vi "GDSIconEditor_CreateVIIcon.vi"(6 "ViRef(IgnoreIfNotWired)":refnum<vi>, 7 "AutomaticUpdateNoQuestionsAsked(False)":bool, 8 "error in (no error)":errorcluster, 9 "Application:Menu Launch:VI":string, 10 "Application:Menu Launch:App":refnum<vi>, 11 "FileNameConverions":T1) -> (0 "error out":errorcluster)   [LabVIEW 2020]
uses:
  <resource>/Framework/Providers/Open_GDS/ClassProviders/Common/LvIcon_class/GDSLvIcon_ColorControl.ctl
  <resource>/Framework/Providers/Open_GDS/ClassProviders/Common/IconEditor/private/GDSIconEditor_FileNameFilter.ctl
  <resource>/Framework/Providers/Open_GDS/ClassProviders/Common/IconEditor/private/GDSIconEditor_ScopeType.ctl
  <vilib>/picture/picture.llb/imagedata.ctl
  <vilib>/Utility/miscctls.llb/LVPoint32TypeDef.ctl
  <resource>/Framework/Providers/Open_GDS/ClassProviders/Provider_LvNativeClass/ClassWriterNative_class/IconSize.ctl
  <resource>/Framework/Providers/Open_GDS/ClassProviders/Common/LvIcon_class/subvis/GDSLvIcon_TextDataType.ctl
  <resource>/Framework/Providers/Open_GDS/ClassProviders/Common/LvIcon_class/GDSLvIcon_WordCompressionType.ctl
  <resource>/Framework/Providers/Open_GDS/ClassProviders/Common/LvIcon_class/GDSLvIcon_TextAlignment.ctl
  <vilib>/event_ctls.llb/lveventtype.ctl
  <vilib>/Utility/miscctls.llb/LVPositionTypeDef.ctl
  <resource>/Framework/Providers/Open_GDS/ClassProviders/Common/IconEditor/private/GDSIconEditor_IconDialog_Input.vi
  <vilib>/Utility/miscctls.llb/LVPointTypeDef.ctl
  <vilib>/Analysis/baseanly.llb/Mean (DBL).vi
  <resource>/Framework/Providers/Open_GDS/ClassProviders/Provider_LvNativeClass/ClassWriterNative_class/ClassWriterNative.lvclass
  <vilib>/Analysis/NI_AALBase.lvlib
panel:
  in  "QuickIcons":u16(ring) items=["<Select an icon>", "Error Wire overlay", "-", "Configure..."]
  in  "ClearIcon":bool
  out "ProductPicture":picture
  out "_IconPreview":picture caption="Icon Preview"
  out "DragIcon":picture
  in  "_MethodIconName":string caption="Body Text"
  in  "FloodFillMask":bool
  out "_IconName":string
  in  "_IconSearchText":string caption="Icon search text"
  in  "_Manage":bool
  in  "_Folders":u16(ring) caption="Folders" items=["<All icons>", "...EW 2020\\resource\\Framework\\Providers\\Icons", "...source\\Framework\\Providers\\Open_GDS\\Glyphs", "...esource\\Framework\\Providers\\Open_GDS\\Icons", "...el.holmstrom\\Documents\\LabVIEW Data\\Glyphs"]
  out "Icons":picture
  in  "_Icons":bool
  in  "_TextAlignment":u16(ring) caption="Text Alignment" items=["Center", "Left", "Right"]
  in  "_IconSize":u16(ring) caption="Icon Size" items=["Full", "1 c-term high", "2 c-term high", "3 c-term high", "4 c-term high"]
  in  "_HelpCreateClass":bool
  out "_FilePrefixFound":string caption="Prefix found"
  in  "_ApplyHeaderToAll":bool caption="Apply this header to all\nVIs/Ctrls in this folder"
  in  "_BodyTextColor":T2 caption="Body Text"
  in  "_BackgroundColor":T2 caption="Body Background"
  in  "_FontCompression":enum16{"Auto", "On", "Off"}(ring) caption="Font Compression"
  in  "_FontCapitalOnly":bool=TRUE caption="Force Capital Letters"
  out "_After":picture caption="New"
  out "_ViNotSavedMessage":string caption="VI not saved. Please select a path!"
  in  "_Cancel":bool
  in  "Accept":bool
  in  "_EditHeader":bool
  in  "_TemplateVI":bool
  in  "_VIPath":path caption="VI Path"
  out "_Before":picture caption="Current"
  out "_Scope":string caption="Visibility"
  in  "_OCR":bool
  in  "_HideHeader":bool=TRUE caption="Force Capital Letters"
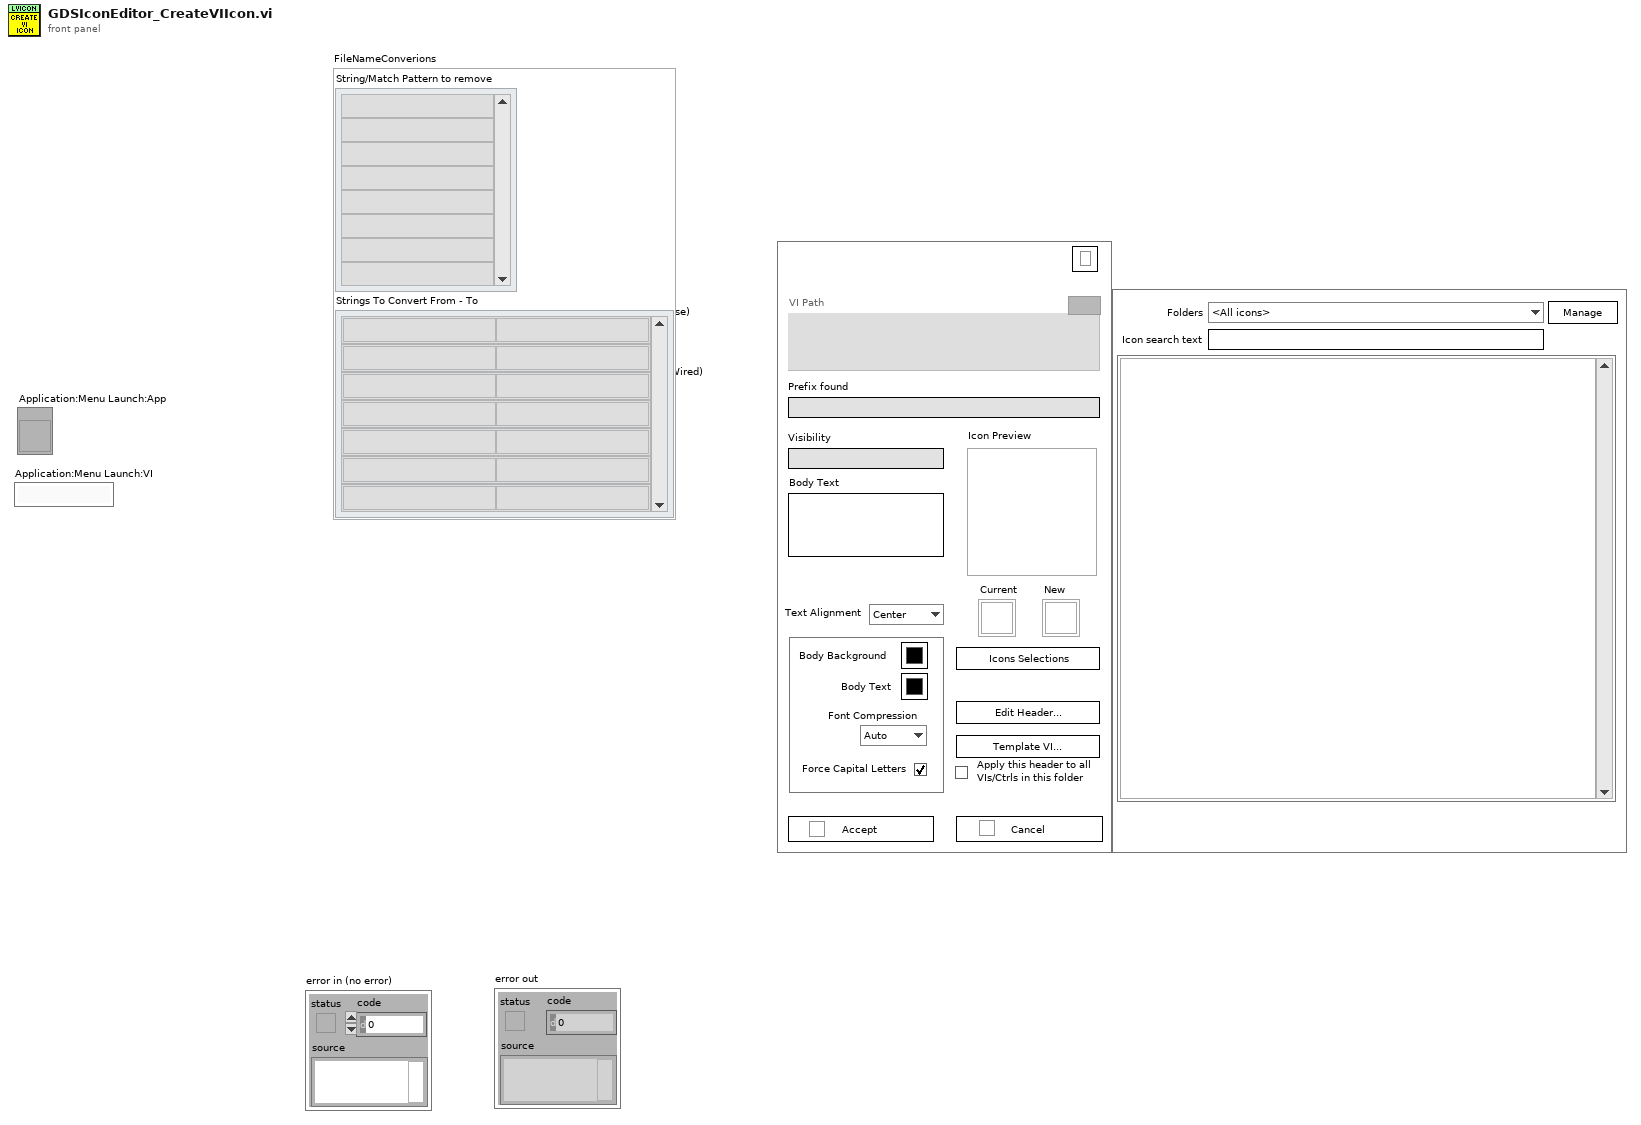
[diagram p1: front panel]
types:
  T1 = typedef "GDSIconEditor_FileNameFilter.ctl" = cluster{"String/Match Pattern to remove":string[], "Strings To Convert From - To":cluster{"From":string, "To":string}[]}
  T2 = typedef "GDSLvIcon_ColorControl.ctl" = cluster{"Decal":bool, "Color":u32}
  T3 = typedef "GDSIconEditor_ScopeType.ctl" = enum16{"Public", "Proteced", "Private"}
  T4 = typedef "imagedata.ctl" = cluster{"image type":i32, "image depth":i32, "image":u8[], "mask":u8[], "colors":u32[], "Rectangle":cluster{"left":i16, "top":i16, "right":i16, "bottom":i16}}
  T5 = typedef "LVPoint32TypeDef.ctl" = cluster{"Horizontal":i32, "Vertical":i32}
  T6 = cluster{"License key":string, "Key info":string, "Prefix":string, "Header exists":bool, "Separator":string, "Folder":path, "VIs":path[], "VI Path":path, "VI exist":bool, "VI name":string, "Icon exist":bool, "ViRef":refnum<vi>, "LibraryRef":refnum<vi>, "Scope":T3, "FrameColor":u32, "Frame thickness":i32, "HeaderIcon":u8[][], "BodyIconHeight":i32, "BodyIconWidth":i32, "IconOut":u8[][], "AppRef":refnum<vi>, "Counter":i32, "Text1":string, "Text2":string, "Text0":string, "Type":enum16{"LvClass", "Library", "X-Control"}, "ConnectorPaneHeight":i32[], "StartRow":i32, "StartIconSize":u16, "Offset":cluster{"X":i32, "Y":i32}, "OldOffset":cluster{"X":i32, "Y":i32}, "Icons":T4[], "IconPos":cluster{"left":i16, "top":i16, "right":i16, "bottom":i16}[], "IconSelected":i32, "BgIcon":u8[][], "BgIconOffset":cluster{"X":i32, "Y":i32}, "Folders":path[], "DraggingIcon":bool, "BodyIcon":u8[][], "BgIconMask":u8[], "HeaderBkColor":u32, "CurrentIcon":cluster{"BgIcon":u8[][], "BgIconOffset":cluster{"X":i32, "Y":i32}, "BgIconMask":u8[], "ColorsOkayforiconToBeOnTopOf":u8[]}, "Moving":bool, "IconDropped":i32, "StartMethodName":string, "DraggingText":bool, "TextBounds":cluster{"FirstRow":i32, "FirstColumn":i32, "LastRow":i32, "LastColumn":i32}, "StartTextDraggingPos":T5, "NoControlsToMove":bool, "LayoutChangeExist":bool, "IconNames":string[], "IconPaths":cluster{i32, "path out":path}[], "Library":bool, "ClassBodyIcon":string, "FirstTime":bool, "TermWindowOpen":bool, "RowStart(0)":i32, "ImageRows(32)":i32, "Splitter0px":bool}
  T7 = typedef "LVBoundsTypeDef.ctl" = cluster{"Width":u32, "Height":u32}
  T8 = typedef "LVRectTypeDef.ctl" = cluster{"Left":i16, "Top":i16, "Right":i16, "Bottom":i16}
  T9 = typedef "ClassWriterNative.lvclass/IconSize.ctl" = enum16{"Full", "1 c-term high", "2 c-term high", "3 c-term high"}
  T10 = typedef "GDSLvIcon_TextDataType.ctl" = cluster{"Text":string, "Allow Only Capital Chars":bool, "Compression":T11, "Alignment":T12}
  T11 = typedef "GDSLvIcon_WordCompressionType.ctl" = enum16{"Auto", "On", "Off"}
  T12 = typedef "GDSLvIcon_TextAlignment.ctl" = enum16{"Center", "Left", "Right"}
  T13 = cluster{"BgIcon":u8[][], "BgIconOffset":cluster{"X":i32, "Y":i32}, "BgIconMask":u8[], "ColorsOkayforiconToBeOnTopOf":u8[]}
  T14 = typedef "lveventtype.ctl" = enum32{"Null", "Timeout", "Annotation Menu Selection", "Annotation Menu Selection?", "App Instance Close", "App Instance Close?", "Autoscale Range Change", "Bookmark Info Change", "Cell Edit", "Cell Edit?", "Cursor Grab", "Cursor Grab?", "Cursor Menu Selection", "Cursor Menu Selection?", "Cursor Move", "Cursor Release", "Data Change", "Direction Change", "Display State Change", "Drag Ended", "Drag Enter", "Drag Leave", "Drag Over", "Drag Source Update", "Drag Starting", "Drag Starting?", "Drop", "Exec State Change", "Key Down", "Key Down?", "Key Repeat", "Key Repeat?", "Key Up", "Listbox Double Click", "Menu Activation?", "Menu Selection (App)", "Menu Selection? (App)", "Menu Selection (User)", "Mouse Down", "Mouse Down?", "Mouse Enter", "Mouse Leave", "Mouse Move", "Mouse Up", "Mouse Wheel", "NI Security User Change (App)", "Pane Size", "Panel Close", "Panel Close?", "Panel Resize", "Plot Attribute Change", "Scale Range Change", "Shortcut Menu Activation?", "Shortcut Menu Selection (App)", "Shortcut Menu Selection? (App)", "Shortcut Menu Selection (User)", "Tree Double Click", "Tree Drag", "Tree Drag?", "Tree Drop", "Tree Drop?", "Tree Item Close", "Tree Item Close?", "Tree Item Open", "Tree Item Open?", "User Event", "Value Change"}
  T15 = typedef "LVPositionTypeDef.ctl" = cluster{"Left":i32, "Top":i32}
  T16 = typedef "GDSIconEditor_IconDialog_Input.vi" = cluster{"HeaderIcon":u8[][], "RowStart(0)":i32, "ImageRows(32)":i32, "FrameThickness(1)":u32, "FrameColor":u32, "IconTextDataType":T10, "BodyTextColor":u32, "BodyBackgroundColor":u32, "BodyIconHeight":i32, "BodyIconWidth":i32, "HeaderBackgroundColor":u32, "BodyIcon":u8[][], "Offset":cluster{"X":i32, "Y":i32}, "CurrentIcon":cluster{"BgIcon":u8[][], "BgIconOffset":cluster{"X":i32, "Y":i32}, "BgIconMask":u8[], "ColorsOkayforiconToBeOnTopOf":u8[]}}
  T17 = typedef "LVPointTypeDef.ctl" = cluster{"Horizontal":i16, "Vertical":i16}
  T18 = enum32{"invalid scope", "public", "private", "protected", "community"}
  T19 = typedef "Librarian File Info Out.ctl" = cluster{"creation date":u32, "last mod date":u32, "type":string, "creator":string, "LV version":i32, "size":i32, "top level":bool}
  T20 = enum32{"invalid VI type", "Standard VI", "Control VI", "Global VI", "Polymorphic VI", "Configuration VI", "SubSystem", "Facade VI", "Method VI", "Statechart Diagram VI"}
  T21 = typedef "GDSLvClass_IconSettingsType.ctl" = cluster{"Frame":u32, "Frame thickness":u8, "Header Background":u32, "Header Text":u32, "ColorPublic":u32, "ColorProtected":u32, "ColorPrivate":u32, "Body Text":u32, "ClassBodyIcon":string}
  T22 = cluster{"CtrlRef":refnum<vi>, "BeforeTerminalIndex":i32, "AfterTerminalIndex":i32}[]
  T23 = cluster{"FirstRow":i32, "FirstColumn":i32, "LastRow":i32, "LastColumn":i32}
  T24 = typedef "ColorControl.ctl" = cluster{"Decal":bool, "Color":u32}
  T25 = typedef "LVMouseTypeDef.ctl" = cluster{"Mouse Position":cluster{"X":i32, "Y":i32}, "Mouse Modifiers":cluster{"Button Down":bool, "Shift Mod":bool, "Menu Mod":bool, "Option Mod":bool}}
  T26 = cluster{"left":i16, "top":i16, "right":i16, "bottom":i16}[]
  T27 = typedef "eventvkey.ctl" = enum16{"ASCII", "Enter", "Return", "Shift", "Ctrl", "Alt", "Cmd", "Opt", "Caps", "NumLock", "Clear", "Break", "Up", "Down", "Left", "Right", "Insert", "Delete", "Home", "End", "PageUp", "PageDown", "Escape", "Help", "Pause", "ScrollLock", "F1", "F2", "F3", "F4", "F5", "F6", "F7", "F8", "F9", "F10", "F11", "F12", "F13", "F14", "F15", "F16", "F17", "F18", "F19", "F20", "F21", "F22", "F23", "F24", "Play", "VolumeUp", "VolumeDown", "Mute", "Two Byte Char"}
  T28 = cluster{"Shift":bool, "Ctrl":bool, "Alt":bool, "Cmd":bool, "Opt":bool}
  T29 = cluster{"left":i16, "top":i16, "right":i16, "bottom":i16}
  T30 = enum32{"existing file", "new file", "new or existing file", "existing dir", "new dir", "new or existing dir", "existing file (use LLBs)", "new file (use LLBs)", "new or existing file (use LLBs)", "new or existing file or directory (use LLBs)", "existing dir (use LLBs)", "new dir (use LLBs)", "new or existing dir (use LLBs)", "existing file or dir", "new file or dir", "new or existing file or dir", "existing file or dir (use LLBs)", "new file or dir (use LLBs)"}
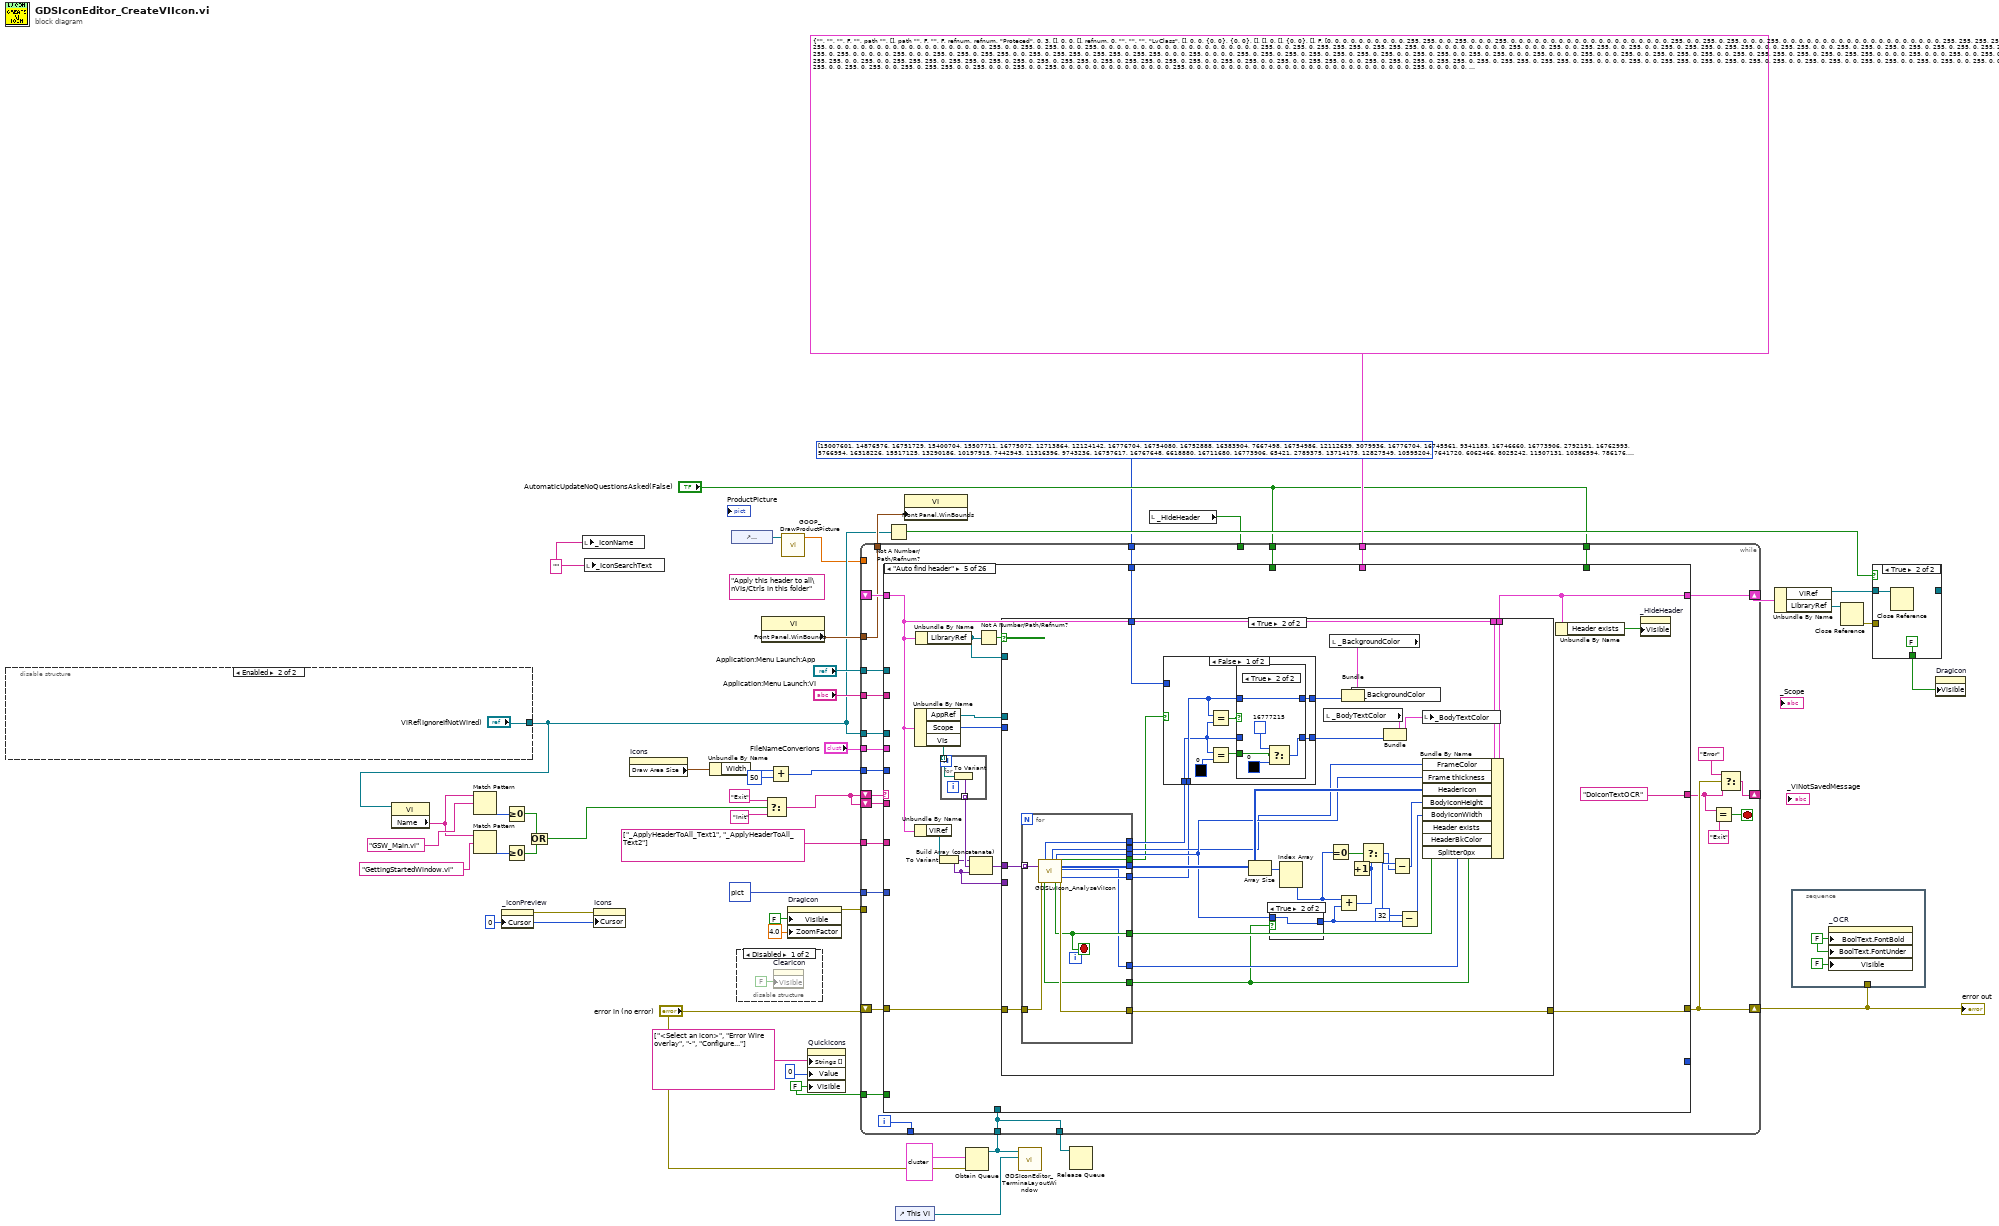
[diagram p0: block diagram]
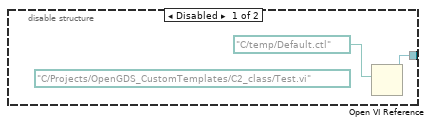
[diagram p3: hidden frame]
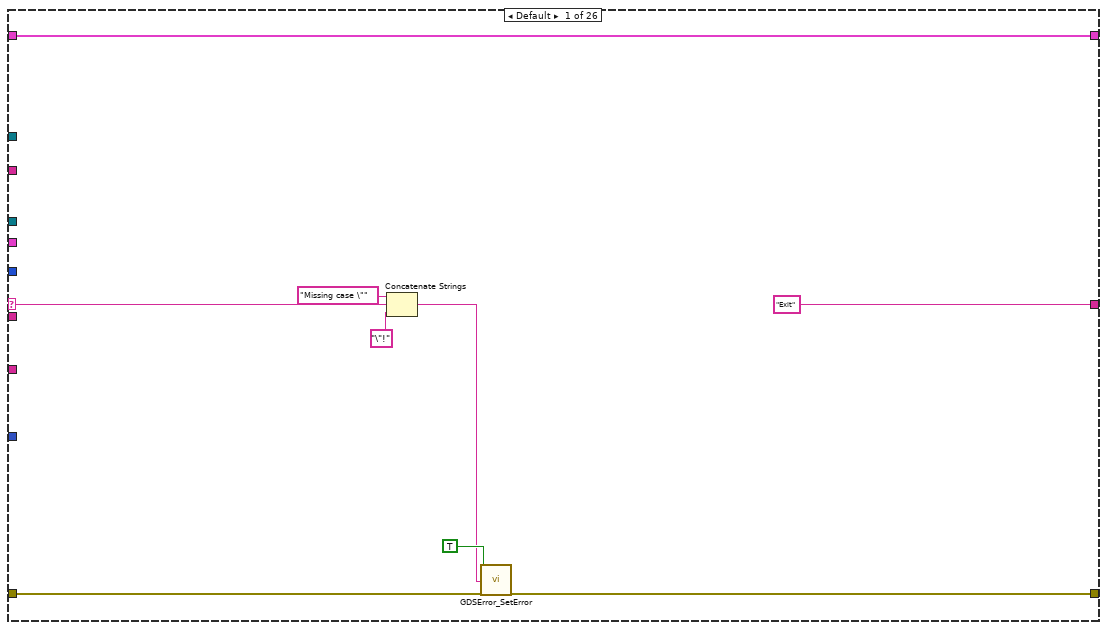
[diagram p5: hidden frame]
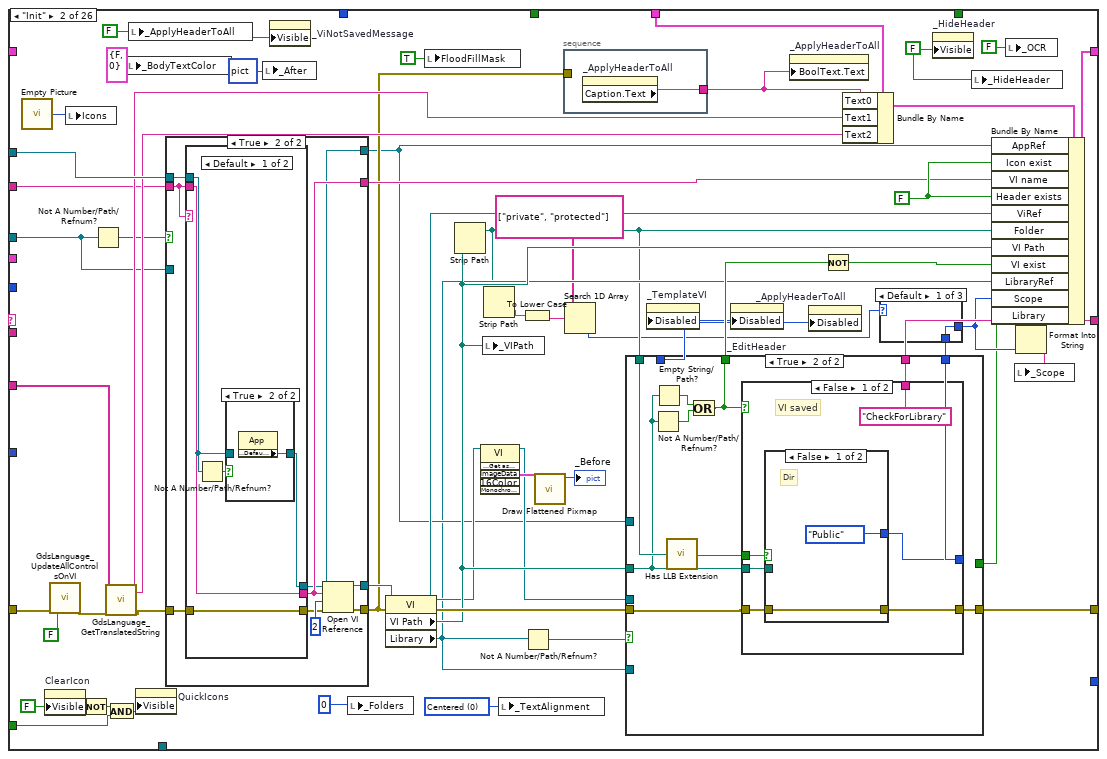
[diagram p6: hidden frame]
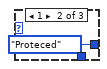
[diagram p7: hidden frame]
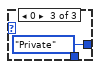
[diagram p8: hidden frame]
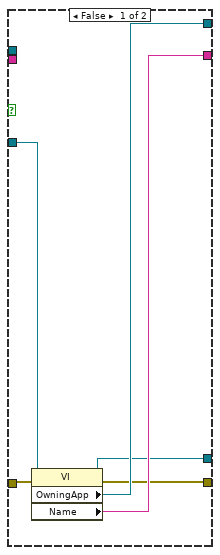
[diagram p9: hidden frame]
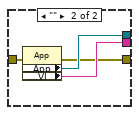
[diagram p11: hidden frame]
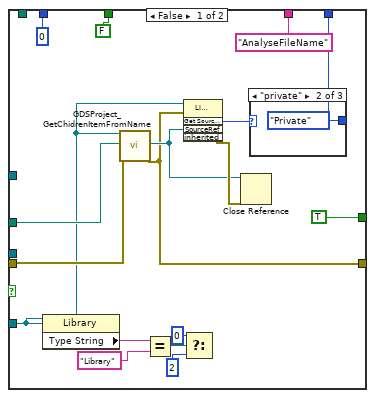
[diagram p12: hidden frame]
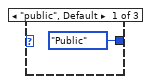
[diagram p13: hidden frame]
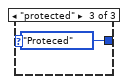
[diagram p14: hidden frame]
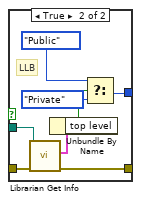
[diagram p15: hidden frame]
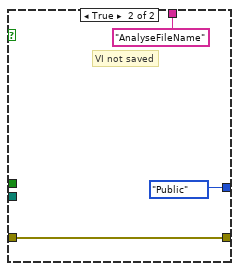
[diagram p16: hidden frame]
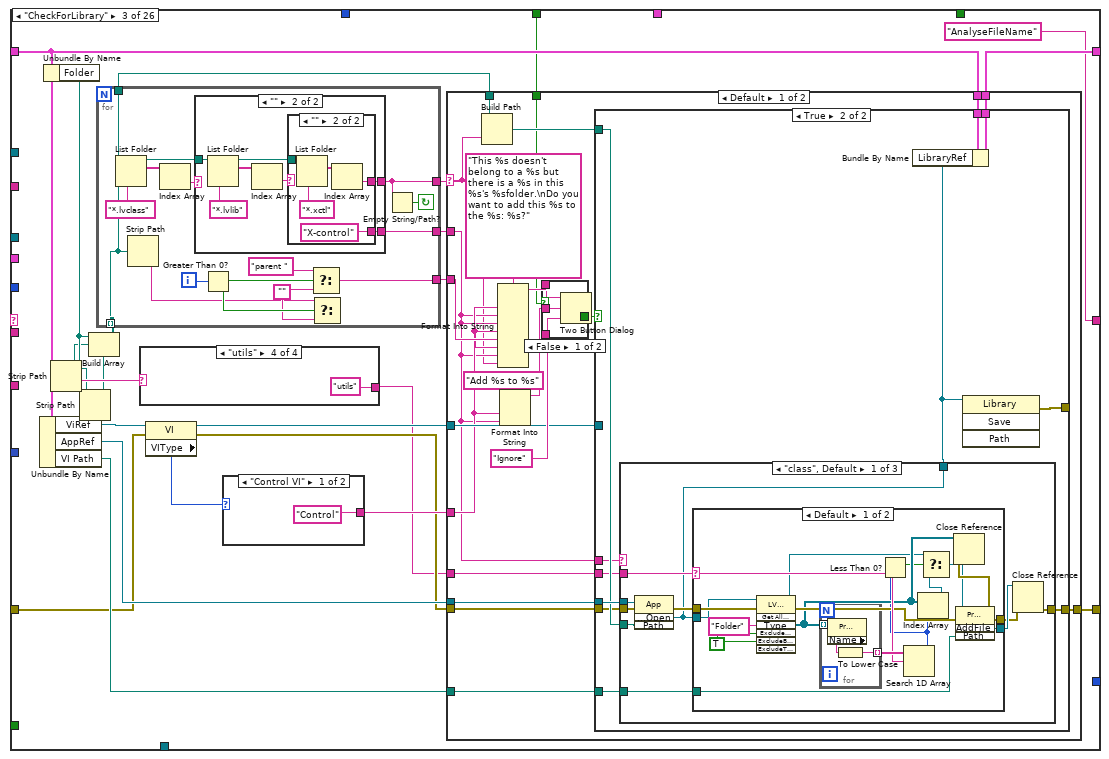
[diagram p17: hidden frame]
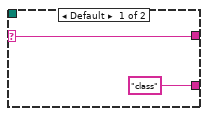
[diagram p18: hidden frame]
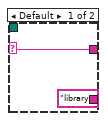
[diagram p19: hidden frame]
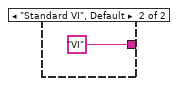
[diagram p20: hidden frame]
diagram:
  w1 = FALSE ("Visible")
  w24 = "" ("_IconSearchText")
  w27 = 0 ("Cursor")
  (unwired) "Apply this header to all\nVIs/Ctrls in this folder" ("Caption.Text")
  n1 = disable-structure shown="Enabled" {
    disable-tunnel: [w52 "ViRef(IgnoreIfNotWired)"] -> w22
    frame Disabled {
      (unwired) path "C:/Projects/OpenGDS_CustomTemplates/C2_class/Test.vi" ("Folder Path")
      n2 = Open VI Reference(vi path=path "C:/temp/Default.ctl" ("Folder Path")) -> (vi reference=w52:refnum<vi>)  [unwired: 5 in, 1 out]
    }
    frame Enabled {
    }
  }
  n3 = property class="VI"(reference=w22) -> ("Name"=w11:string)  [unwired: 1 in, 2 out]
  n4 = Match Pattern(string=w11, regular expression="GSW_Main.vi" ("y")) -> (offset past match=w13:i32)  [unwired: 1 in, 3 out]
  n5 = Match Pattern(string=w11, regular expression="GettingStartedWindow.vi" ("y")) -> (offset past match=w12:i32)  [unwired: 1 in, 3 out]
  n6 = property on="_IconPreview" class="Pict"("Cursor"=w27) -> (error out=w26:errorcluster)  [unwired: 2 in, 1 out]
  n7 = Greater Or Equal To 0?(x=w13) -> (x >= 0?=w8:bool)
  n8 = Greater Or Equal To 0?(x=w12) -> (x >= 0?=w9:bool)
  n9 = Or(x=w8, y=w9) -> (x .or. y?=w18:bool)
  n10 = local write "_IconName"(w24) -> ()
  n11 = local write "_IconSearchText"(w24) -> ()
  n12 = property on="Icons" class="Pict"(error in=w26, "Cursor"=w27) -> ()  [unwired: 1 in, 2 out]
  n13 = property on="Icons" class="Pict"() -> ("Draw Area Size"=w33:T7)  [unwired: 2 in, 2 out]
  n14 = Unbundle By Name(w33) -> ("Width"=w35:u32)
  n15 = control-ref of="ProductPicture"() -> (w6:refnum<vi>)
  n16 = disable-structure shown="Disabled" {
    frame Disabled {
      n17 = property on="ClearIcon" class="Bool"("Visible"=FALSE) -> ()  [unwired: 2 in, 2 out]
    }
    frame Enabled {
    }
  }
  n18 = property class="VI"() -> ("Front Panel.WinBounds"=w25:T8)  [unwired: 2 in, 2 out]
  n19 = Select(t="Exit", s=w18, f="Init") -> (s? t:f=w19:string)
  n20 = Add(x=w35, y=u32 50) -> (x+y=w34:u32)
  n21 = call <resource>:"GOOP_DrawProductPicture.vi"("ProductPictureControl"=w6) -> ("Zoom Factor"=w5:sgl)  [unwired: 10 in]
  n22 = property on="DragIcon" class="Pict"("Visible"=FALSE, "ZoomFactor"=sgl 4.0 ("Zoom Factor")) -> (error out=w30:errorcluster)  [unwired: 2 in, 1 out]
  n23 = property on="QuickIcons" class="Ring (strict)"("Strings []"=string[] ["<Select an icon>", "Error Wire overlay", "-", "Configure..."], "Value"=0, "Visible"=w1) -> ()  [unwired: 2 in, 2 out]
  n24 = Not A Number/Path/Refnum?(number/path/refnum=w22) -> (NaN/Path/Refnum?=w43:bool)
  n25 = control-ref of="This VI"() -> (w37:refnum<vi>)
  n26 = Obtain Queue(element data type=cluster{"Message":string, "Picture":picture} {"Message"="", "Picture"=bytes[0]} ("Message"), error in (no error)="error in (no error)") -> (queue out=w38:refnum<queue>)  [unwired: 3 in, 2 out]
  n27 = call <resource>:"GDSIconEditor_TerminaLayoutWindow.vi"("ViRef"=w37, "ControlQueue"=w38) -> ()  [unwired: 10 in]
  n28 = local read "_HideHeader"() -> (w7:bool)
  n29 = while {
    tunnel: picture bytes[1054] ("Icon not available") -> [w76]
    shift-left: "error in (no error)" -> [w79]
    shift-right: [w71] -> w23
    shift-left: _ -> [w77]
    shift-right: [w78] -> w49
    shift-left: w19 -> [w80]
    shift-right: [w70] -> _
    tunnel: "Application:Menu Launch:App" -> [w75]
    tunnel: "Application:Menu Launch:VI" -> [w74]
    tunnel: T6 {"License key"="", "Key info"="", "Prefix"="", "Header exists"=FALSE, "Separator"="", "Folder"=path "", "VIs"=[], "VI Path"=path "", "VI exist"=FALSE, "VI name"="", "Icon exist"=FALSE, "ViRef"=refnum, "LibraryRef"=refnum, "Scope"=enum."Proteced", "FrameColor"=0, "Frame thickness"=3, "HeaderIcon"=[], "BodyIconHeight"=0, "BodyIconWidth"=0, "IconOut"=[], "AppRef"=refnum, "Counter"=0, "Text1"="", "Text2"="", "Text0"="", "Type"=enum."LvClass", "ConnectorPaneHeight"=[], "StartRow"=0, "StartIconSize"=0, "Offset"={"X"=0, "Y"=0}, "OldOffset"={"X"=0, "Y"=0}, "Icons"=[], "IconPos"=[], "IconSelected"=0, "BgIcon"=[], "BgIconOffset"={"X"=0, "Y"=0}, "Folders"=[], "DraggingIcon"=FALSE, "BodyIcon"=[[0, 0, 0, 0, 0, 0, 0, 0, 0, 0, 255, 255, 0, 0, 255, 0, 0, 0, 255, 0, 0, 0, 0, 0, 0, 0, 0, 0, 0, 0], [0, 0, 0, 0, 0, 0, 0, 0, 0, 255, 0, 0, 255, 0, 255, 0, 0, 0, 255, 0, 0, 0, 0, 0, 0, 0, 0, 0, 0, 0], [0, 0, 0, 0, 0, 0, 0, 0, 0, 255, 255, 255, 255, 0, 255, 0, 0, 0, 255, 0, 0, 0, 0, 0, 0, 0, 0, 0, 0, 0], [0, 0, 0, 0, 0, 0, 0, 0, 0, 255, 0, 0, 255, 0, 255, 0, 0, 0, 255, 0, 0, 0, 0, 0, 0, 0, 0, 0, 0, 0], [0, 0, 0, 0, 0, 0, 0, 0, 0, 255, 0, 0, 255, 0, 255, 255, 255, 0, 255, 255, 255, 0, 0, 0, 0, 0, 0, 0, 0, 0], [0, 0, 255, 0, 0, 0, 255, 0, 0, 255, 255, 0, 0, 255, 0, 0, 255, 0, 255, 255, 0, 255, 255, 0, 0, 0, 255, 255, 0, 0], [0, 255, 0, 255, 0, 255, 0, 255, 0, 255, 0, 255, 0, 255, 255, 0, 255, 0, 255, 0, 0, 255, 0, 255, 0, 255, 0, 0, 0, 0], [0, 255, 0, 0, 0, 255, 0, 255, 0, 255, 255, 0, 0, 255, 0, 255, 255, 0, 255, 255, 0, 255, 255, 0, 0, 0, 255, 0, 0, 0], [0, 255, 0, 255, 0, 255, 0, 255, 0, 255, 0, 255, 0, 255, 0, 0, 255, 0, 255, 0, 0, 255, 0, 255, 0, 0, 0, 255, 0, 0], [0, 0, 255, 0, 0, 0, 255, 0, 0, 255, 0, 255, 0, 255, 0, 0, 255, 0, 255, 255, 0, 255, 0, 255, 0, 255, 255, 0, 0, 0], [0, 255, 0, 0, 0, 255, 0, 0, 255, 0, 0, 255, 0, 255, 0, 0, 255, 0, 255, 255, 0, 0, 255, 0, 0, 255, 255, 255, 0, 255], [255, 0, 255, 0, 255, 0, 255, 0, 255, 255, 0, 255, 0, 255, 255, 0, 255, 0, 255, 0, 0, 255, 0, 255, 0, 0, 255, 0, 0, 255], [255, 0, 0, 0, 255, 0, 255, 0, 255, 0, 255, 255, 0, 255, 0, 255, 255, 0, 255, 255, 0, 255, 0, 0, 0, 0, 255, 0, 0, 255], [255, 0, 255, 0, 255, 0, 255, 0, 255, 0, 0, 255, 0, 255, 0, 0, 255, 0, 255, 0, 0, 255, 0, 255, 0, 0, 255, 0, 0, 255], [0, 255, 0, 0, 0, 255, 0, 0, 255, 0, 0, 255, 0, 255, 0, 0, 255, 0, 255, 255, 0, 0, 255, 0, 0, 0, 255, 0, 0, 255], [0, 0, 0, 0, 0, 0, 0, 0, 0, 0, 0, 0, 0, 0, 255, 0, 0, 0, 0, 0, 0, 0, 0, 0, 0, 0, 0, 0, 0, 0], [0, 0, 0, 0, 0, 0, 0, 0, 0, 0, 0, 0, 0, 255, 0, 0, 0, 0, 0, 0, 0, 0, 0, 0, 0, 0, 0, 0, 0, 0], [0, 0, 0, 0, 0, 0, 0, 0, 0, 0, 0, 0, 0, 255, 255, 0, 0, 0, 0, 0, 0, 0, 0, 0, 0, 0, 0, 0, 0, 0], [0, 0, 0, 0, 0, 0, 0, 0, 0, 0, 0, 0, 0, 255, 0, 255, 0, 0, 0, 0, 0, 0, 0, 0, 0, 0, 0, 0, 0, 0], [0, 0, 0, 0, 0, 0, 0, 0, 0, 0, 0, 0, 0, 0, 255, 0, 0, 0, 0, 0, 0, 0, 0, 0, 0, 0, 0, 0, 0, 0], [0, 0, 0, 0, 0, 0, 0, 0, 0, 0, 0, 0, 0, 0, 0, 0, 0, 0, 0, 0, 0, 0, 0, 0, 0, 0, 0, 0, 0, 0], [0, 0, 0, 0, 0, 0, 0, 0, 0, 0, 0, 0, 0, 0, 0, 0, 0, 0, 0, 0, 0, 0, 0, 0, 0, 0, 0, 0, 0, 0]], "BgIconMask"=[], "HeaderBkColor"=0, "CurrentIcon"={"BgIcon"=[], "BgIconOffset"={"X"=0, "Y"=0}, "BgIconMask"=[], "ColorsOkayforiconToBeOnTopOf"=[]}, "Moving"=FALSE, "IconDropped"=-1, "StartMethodName"="", "DraggingText"=FALSE, "TextBounds"={"FirstRow"=2, "FirstColumn"=1, "LastRow"=6, "LastColumn"=27}, "StartTextDraggingPos"={"Horizontal"=0, "Vertical"=0}, "NoControlsToMove"=FALSE, "LayoutChangeExist"=FALSE, "IconNames"=[], "IconPaths"=[], "Library"=FALSE, "ClassBodyIcon"="", "FirstTime"=TRUE, "TermWindowOpen"=FALSE, "RowStart(0)"=0, "ImageRows(32)"=32, "Splitter0px"=FALSE} ("Local data") -> [w67]
    shift-left: w19 -> [w66]
    tunnel: string[] ["_ApplyHeaderToAll_Text1", "_ApplyHeaderToAll_Text2"] -> [w65]
    tunnel: w22 -> [w64]
    tunnel: w38 -> [w63]
    tunnel: [w63] -> w39
    tunnel: w34 -> [w62]
    tunnel: w25 -> [w61]
    tunnel: [w61] -> w32
    tunnel: w30 -> [_]
    tunnel: [w60] -> _
    tunnel: "AutomaticUpdateNoQuestionsAsked(False)" -> [w59]
    tunnel: "AutomaticUpdateNoQuestionsAsked(False)" -> [w58]
    tunnel: u32[] [15007601, 14876576, 16751729, 15400704, 15507711, 16775072, 12713864, 12124142, 16776704, 16754080, 16752888, 16383904, 7667498, 16754986, 12112639, 3079936, 16776704, 16745561, 9341183, 16746660, 16773906, 2792191, 16762993, 5766954, 16318226, 15517125, 13290186, 10197915, 7442943, 11316396, 9743236, 16757617, 16767648, 6618880, 16711680, 16773906, 65421, 2789375, 13714175, 12827549, 10595204, 7641720, 6062466, 8025242, 11507131, 10386594, 786176, 8584960, 16318208, 16731648, 16755616, 16734715, 14399157, 16754801, 16714752, 10026888, 3524608] -> [w57]
    tunnel: w7 -> [_]
    tunnel: w5 -> [_]
    tunnel: "FileNameConverions" -> [w56]
    tunnel: w1 -> [w55]
    i -> [w60]
    stop <- w73 stop-if-true
    n30 = case shown="\"Auto find header\"" w80 {
      selector: w80 -> [w82 _ _ _ _ _ w824 _ _ w957 _ _ _ w1613 _ _ _ w1794 _ _ _ _ _ _ _ _]
      tunnel: ["Exit" w111 "AnalyseFileName" "Auto find header" "DoIconTextOCR" "DoIconTextOCR_Before" ("t") w819 "Generate icon" "ShowLayoutChange" ("item tag") w976 w1021 w1096 "UpdateIcon" ("y") w1620 "ReadIcons" "Generate icon" "DrawIcons" ("y") "Idle" ("y") "Idle" ("y") "Exit" w1950 "Auto find header" w2015 "Exit" ("y") w2079 "Exit" ("y")] -> w69
      tunnel: w79 -> [w89 w126 w233 w424 w539 w767 w828 w843 w877 w956 w1039 w1067 w1594 w1648 w1680 w1745 w1756 w1804 w1929 w1940 w1961 w2000 w2023 w2048 w2081 w2131]
      tunnel: [w88 w140 w232 w431 w540 w792 w829 w842 w876 w953 w1038 w1066 w1594 w1648 w1679 w1745 w1751 w1806 w1929 w1937 w1962 w2001 w2008 w2047 w2080 w2131] -> w71
      tunnel: [w85 w144 w246 w430 w529 w793 w816 w840 w873 w960 w1024 w1082 w1596 w1617 w1689 w1746 w1761 w1819 w1925 w1941 w1964 w1997 w2011 w2052 w2076 w2130] -> w78
      tunnel: w77 -> [w85 _ w242 w423 w536 w791 w817 w841 w874 w961 w1025 w1083 w1597 w1617 w1690 w1747 w1759 w1807 w1932 w1941 w1963 w2002 w2011 w2052 w2077 w2130]
      tunnel: w76 -> [_ _ _ _ _ _ _ _ _ _ _ _ _ _ _ _ _ _ _ _ _ _ _ _ _ _]
      tunnel: w75 -> [_ w136 _ _ _ _ _ _ _ _ _ _ _ _ _ _ _ _ _ _ _ _ _ _ _ _]
      tunnel: w74 -> [_ w117 _ _ _ _ _ _ _ _ _ _ _ _ _ _ _ _ _ _ _ _ _ _ _ _]
      tunnel: w67 -> [_ w119 _ _ _ _ _ _ _ _ _ _ _ _ _ _ _ _ _ _ _ _ _ _ _ _]
      tunnel: w66 -> [_ _ _ _ _ _ _ _ _ _ _ _ _ _ _ _ _ _ _ _ _ _ _ _ _ w2132]
      tunnel: w65 -> [_ w123 _ _ _ _ _ _ _ _ _ _ _ _ _ _ _ _ _ _ _ _ _ _ _ _]
      tunnel: w64 -> [_ w112 _ _ _ _ _ _ _ _ _ _ _ _ _ _ _ _ _ _ _ _ _ _ _ _]
      tunnel: w63 -> [_ _ _ _ _ _ _ _ _ _ w1037 w1071 _ _ _ _ _ _ _ _ _ _ _ _ _ _]
      tunnel: w62 -> [_ _ _ _ _ _ _ _ _ _ _ w1072 _ _ _ _ _ _ _ _ _ _ _ _ _ _]
      tunnel: [_ _ _ _ _ _ _ _ _ w950 _ _ _ _ _ _ _ _ _ _ _ _ _ _ _ _] -> _
      tunnel: w59 -> [_ _ w224 _ _ _ _ _ _ _ _ _ _ _ _ _ _ _ _ _ _ _ _ _ _ _]
      tunnel: w58 -> [_ _ _ _ _ _ _ _ _ w949 w1020 _ _ _ _ _ _ _ _ _ _ _ _ _ _ _]
      tunnel: w57 -> [_ _ _ _ w527 w760 _ _ _ _ _ _ _ _ _ _ _ _ _ _ _ _ _ _ _ _]
      tunnel: w56 -> [_ _ _ w418 _ _ _ _ _ _ _ _ _ _ _ _ _ _ _ _ _ _ _ _ _ _]
      tunnel: w55 -> [_ w90 _ _ _ _ _ _ _ _ _ w1065 _ _ _ _ _ _ _ _ _ _ _ _ _ _]
      frame Default {
        n31 = Concatenate Strings("Missing case \"" ("source"), w82, "\"!") -> (w81:string)
        n32 = call <resource>:"GDSError_SetError.vi"("status"=TRUE, "source"=w81, "error in (no error)"=w89) -> ("error out"=w88:errorcluster)  [unwired: 16 in]
      }
      frame "Init" {
        w93 = FALSE ("Visible")
        w94 = FALSE ("_OCR")
        w108 = u16 0 items=["Centered", "Left", "Right"] ("_TextAlignment")
        w106 = FALSE ("ApplyToAll")
        w139 = FALSE ("Header exists")
        n33 = call "Empty Picture"() -> ("empty picture"=w105:picture)
        n34 = property on="ClearIcon" class="Bool"("Visible"=w93) -> ()  [unwired: 2 in, 2 out]
        n35 = call <resource>:"GdsLanguage_UpdateAllControlsOnVI.vi"("error in (no error)"=w126, "CreateLanguageFile(Use this to create a languageFile)"=FALSE) -> ("error out"=w124:errorcluster)  [unwired: 16 in, 1 out]
        n36 = local write "Icons"(w105) -> ()
        n37 = Not(x=w93) -> (.not. x?=w92:bool)
        n38 = Not A Number/Path/Refnum?(number/path/refnum=w112) -> (NaN/Path/Refnum?=w114:bool)
        n39 = call <resource>:"GdsLanguage_GetTranslatedString.vi"("StringID(s)"=w123, "error in (no error)"=w124) -> ("FirstStringOut"=w121:string, "SecondStringOut"=w120:string, "error out"=w118:errorcluster)  [unwired: 14 in, 1 out]
        n40 = And(x=w92, y=w90) -> (x .and. y?=w91:bool)
        n41 = local write "_BodyTextColor"(T2 {"Decal"=FALSE, "Color"=0} ("BodyText")) -> ()
        n42 = local write "_ApplyHeaderToAll"(w106) -> ()
        n43 = property on="QuickIcons" class="Ring (strict)"("Visible"=w91) -> ()  [unwired: 2 in, 2 out]
        n44 = case shown="True" w114 {
          tunnel: [w149 w161] -> w143
          tunnel: [w150 w160] -> w138
          tunnel: w136 -> [_ w158]
          tunnel: [w151 w157] -> w113
          tunnel: w118 -> [w153 w156]
          tunnel: w117 -> [_ w155]
          tunnel: [w148 w154] -> w116
          tunnel: w112 -> [w152 _]
          frame False {
            n45 = property class="VI"(reference=w152, error in=w153) -> (reference out=w149:refnum<vi>, error out=w148:errorcluster, "OwningApp"=w151:refnum<vi>, "Name"=w150:string)
          }
          frame True {
            n46 = case shown="Default" w155 {
              tunnel: [w163 w173] -> w157
              tunnel: [w167 w172] -> w160
              tunnel: [w166 w171] -> w159
              tunnel: w156 -> [w166 w170]
              tunnel: w158 -> [w164 _]
              tunnel: w155 -> [w167 _]
              frame Default {
                n47 = Not A Number/Path/Refnum?(number/path/refnum=w164) -> (NaN/Path/Refnum?=w165:bool)
                n48 = case shown="True" w165 {
                  tunnel: w164 -> [w168 _]
                  tunnel: [w168 w169] -> w163
                  frame False {
                  }
                  frame True {
                    n49 = property class="App"() -> ("App.DefaultApplication"=w169:refnum<vi>)  [unwired: 2 in, 2 out]
                  }
                }
              }
              frame "" {
                n50 = property class="App"(error in=w170) -> (error out=w171:errorcluster, "Application:Menu Launch:App"=w173:refnum<vi>, "Application:Menu Launch:VI"=w172:string)  [unwired: 1 in, 1 out]
              }
            }
            n51 = Open VI Reference(application reference (local)=w157, vi path=w160, options=2, error in (no error)=w159) -> (vi reference=w161:refnum<vi>, error out=w154:errorcluster)  [unwired: 2 in]
          }
        }
        n52 = local write "_After"(picture bytes[1054] ("After")) -> ()
        n53 = property on="_ViNotSavedMessage" class="Str"("Visible"=w106) -> ()  [unwired: 2 in, 2 out]
        n54 = local write "_Folders"(0) -> ()
        n55 = property class="VI"(reference=w143, error in=w116) -> (reference out=w130:refnum<vi>, error out=w137:errorcluster, "VI Path"=w135:path, "Library"=w110:refnum<vi>)
        n56 = local write "FloodFillMask"(TRUE ("FloodFillMask")) -> ()
        n57 = Strip Path(path=w135) -> (stripped path=w102:path)  [unwired: 1 out]
        n58 = invoke class="VI" method="VI Icon.Get as Image Data"(reference=w130) -> (reference out=w129:refnum<vi>, "ImageData"=w132:T4)  [unwired: 5 in, 4 out]
        n59 = local write "_VIPath"(w135) -> ()
        n60 = Strip Path(path=w102) -> (name=w101:string)  [unwired: 1 out]
        n61 = local write "_TextAlignment"(w108) -> ()
        n62 = To Lower Case(string=w101) -> (all lower case string=w104:string)
        n63 = Not A Number/Path/Refnum?(number/path/refnum=w110) -> (NaN/Path/Refnum?=w109:bool)
        n64 = call <vilib>:"Draw Flattened Pixmap.vi"("image data"=w132) -> ("new picture"=→"_Before":picture)  [unwired: 8 in]
        n65 = stacked-sequence {
          tunnel: [w174] -> w115
          tunnel: w116 -> [_]
          frame #0 {
            n66 = property on="_ApplyHeaderToAll" class="Bool (strict)"() -> ("Caption.Text"=w174:string)  [unwired: 2 in, 2 out]
          }
        }
        n67 = Search 1D Array(1D array=string[] ["private", "protected"], element=w104) -> (index of element=w100:i32)  [unwired: 1 in]
        n68 = case shown="True" w109 {
          tunnel: [FALSE ("Cleared?") w197] -> w141
          tunnel: [w184 w204] -> w140
          tunnel: [w187 w202] -> w99
          tunnel: w102 -> [_ w198]
          tunnel: w137 -> [w189 w201]
          tunnel: w135 -> [w190 w196]
          tunnel: w129 -> [_ _]
          tunnel: w110 -> [w182 _]
          tunnel: [u8 0 ("t") _] -> w127
          tunnel: w113 -> [_ _]
          tunnel: ["AnalyseFileName" w195] -> w111
          tunnel: [TRUE ("Cleared?") _] -> w97
          frame False {
            n69 = property class="Library"(reference=w182) -> ("Type String"=w181:string)  [unwired: 1 in, 2 out]
            n70 = call <resource>:"GDSProject_GetChidrenItemFromName.vi"("ProjectItemToSearchFrom"=w182, "ItemToSearchForInProjectTreeBasedOnPath(used if wired)"=w190, "error in (no error)"=w189) -> ("ProjectItemFound"=w185:refnum<vi>, "error out"=w184:errorcluster)  [unwired: 13 in, 2 out]
            n71 = Equal?(x=w181, y="Library") -> (x = y?=w179:bool)
            n72 = invoke class="Library" method="Get Source Scope"(reference=w182, error in=w184, "SourceRef"=w185) -> (error out=w186:errorcluster, "GetSourceScope"=w188:T18)  [unwired: 2 in, 3 out]
            n73 = Select(t=u8 0, s=w179, f=u8 2 ("Disabled")) -> ()  [unwired: 1 out]
            n74 = Close Reference(reference=w185, error in (no error)=w186) -> ()  [unwired: 1 out]
            n75 = case shown="\"private\"" w188 {
              tunnel: [GDSIconEditor_ScopeType."Public" ("Scope") GDSIconEditor_ScopeType."Private" ("Scope") GDSIconEditor_ScopeType."Proteced" ("Scope")] -> w187
              frame "public", Default {
              }
              frame "private" {
              }
              frame "protected" {
              }
            }
          }
          frame True {
            n76 = Not A Number/Path/Refnum?(number/path/refnum=w196) -> (NaN/Path/Refnum?=w199:bool)
            n77 = Empty String/Path?(string/path=w196) -> (empty?=w200:bool)
            n78 = call <vilib>:"Has LLB Extension.vi"("path"=w198) -> ("path to VI library?"=w203:bool)
            n79 = Or(x=w200, y=w199) -> (x .or. y?=w197:bool)
            n80 = case shown="False" w197 {
              tunnel: w201 -> [w210 w223]
              tunnel: [w206 w223] -> w204
              tunnel: w196 -> [w209 _]
              tunnel: w203 -> [w208 _]
              tunnel: [w207 GDSIconEditor_ScopeType."Public" ("Scope")] -> w202
              tunnel: ["CheckForLibrary" "AnalyseFileName"] -> w195
              frame False {
                # "VI saved"
                n81 = case shown="False" w208 {
                  tunnel: w210 -> [w212 w220]
                  tunnel: [w212 w219] -> w206
                  tunnel: w209 -> [_ w218]
                  tunnel: [GDSIconEditor_ScopeType."Public" ("Scope") w216] -> w207
                  frame False {
                    # "Dir"
                  }
                  frame True {
                    # "LLB"
                    n82 = call <vilib>:"Librarian Get Info.vi"("error in (no error)"=w220, "path"=w218) -> ("error out"=w219:errorcluster, "file information"=w217:T19)  [unwired: 7 in, 1 out]
                    n83 = Unbundle By Name(w217) -> ("top level"=w215:bool)
                    n84 = Select(t=GDSIconEditor_ScopeType."Public" ("Scope"), s=w215, f=GDSIconEditor_ScopeType."Private" ("Scope")) -> (s? t:f=w216:T3)
                  }
                }
              }
              frame True {
                # "VI not saved"
              }
            }
          }
        }
        n85 = property on="_TemplateVI" class="Bool"("Disabled"=w127) -> ()  [unwired: 2 in, 2 out]
        n86 = property on="_EditHeader" class="Bool"("Disabled"=w127) -> ()  [unwired: 2 in, 2 out]
        n87 = property on="_ApplyHeaderToAll" class="Bool (strict)"("BoolText.Text"=w115) -> ()  [unwired: 2 in, 2 out]
        n88 = property on="_ApplyHeaderToAll" class="Bool (strict)"("Disabled"=w127) -> ()  [unwired: 2 in, 2 out]
        n89 = Not(x=w141) -> (.not. x?=w142:bool)
        n90 = Bundle By Name(cluster=w119, "Text0"=w115, "Text1"=w121, "Text2"=w120) -> (w122:T6)
        n91 = case shown="Default" w100 {
          tunnel: w99 -> [w145 _ _]
          tunnel: [w145 GDSIconEditor_ScopeType."Proteced" ("Scope") GDSIconEditor_ScopeType."Private" ("Scope")] -> w98
          frame Default {
          }
          frame 1 {
          }
          frame 0 {
          }
        }
        n92 = property on="_HideHeader" class="Bool (strict)"("Visible"=w94) -> ()  [unwired: 2 in, 2 out]
        n93 = local write "_HideHeader"(w94) -> ()
        n94 = Bundle By Name(cluster=w122, "AppRef"=w113, "Icon exist"=w139, "VI name"=w138, "Header exists"=w139, "ViRef"=w130, "Folder"=w102, "VI Path"=w135, "VI exist"=w142, "LibraryRef"=w110, "Scope"=w98, "Library"=w97) -> (w144:T6)
        n95 = local write "_OCR"(FALSE ("_OCR")) -> ()
        n96 = Format Into String(w98) -> (resulting string=w134:string)  [unwired: 3 in, 1 out]
        n97 = local write "_Scope"(w134) -> ()
      }
      frame "CheckForLibrary" {
        n98 = Unbundle By Name(w242) -> ("ViRef"=w241:refnum<vi>, "AppRef"=w236:refnum<vi>, "VI Path"=w235:path)
        n99 = Unbundle By Name(w242) -> ("Folder"=w230:path)
        n100 = Strip Path(path=w230) -> (stripped path=w226:path, name=w244:string)
        n101 = Strip Path(path=w226) -> (stripped path=w225:path)  [unwired: 1 out]
        n102 = Build Array(w230, w226, w225) -> (w229:path[])
        n103 = for {
          tunnel: [w254] -> w243
          tunnel: [w256] -> w238
          tunnel: w229 -> [w255] mode=indexing
          tunnel: [w255] -> w228
          tunnel: [w250] -> w227
          i -> [w252]
          stop <- w253 continue-if-true
          w248 = ""
          n104 = List Folder(path=w255, pattern="*.lvclass") -> (path out=w257:path, filenames=w259:string[])  [unwired: 2 in, 2 out]
          n105 = Strip Path(path=w255) -> (name=w247:string)  [unwired: 1 out]
          n106 = Index Array(array=w259) -> (element=w258:string)  [unwired: 1 in]
          n107 = case shown="\"\"" w258 {
            selector: w258 -> [w262 _]
            tunnel: w257 -> [_ w267]
            tunnel: [w262 w264] -> w254
            tunnel: ["class" ("pattern") w263] -> w256
            frame Default {
            }
            frame "" {
              n108 = List Folder(path=w267, pattern="*.lvlib") -> (path out=w265:path, filenames=w269:string[])  [unwired: 2 in, 2 out]
              n109 = Index Array(array=w269) -> (element=w266:string)  [unwired: 1 in]
              n110 = case shown="\"\"" w266 {
                selector: w266 -> [w271 _]
                tunnel: w265 -> [_ w274]
                tunnel: [w271 w273] -> w264
                tunnel: ["library" ("pattern") "X-control" ("pattern")] -> w263
                frame Default {
                }
                frame "" {
                  n111 = List Folder(path=w274, pattern="*.xctl") -> (filenames=w275:string[])  [unwired: 2 in, 3 out]
                  n112 = Index Array(array=w275) -> (element=w273:string)  [unwired: 1 in]
                }
              }
            }
          }
          n113 = Greater Than 0?(x=w252) -> (x > 0?=w249:bool)
          n114 = Select(t="parent " ("pattern"), s=w249, f=w248) -> (s? t:f=w250:string)
          n115 = Select(t=w247, s=w249, f=w248) -> ()  [unwired: 1 out]
          n116 = Empty String/Path?(string/path=w254) -> (empty?=w253:bool)
        }
        n117 = case shown="\"utils\"" w244 {
          tunnel: [_ "private" ("Type") "protected" ("Type") "utils" ("Type")] -> w231
          frame Default {
          }
          frame "private" {
          }
          frame "protected" {
          }
          frame "utils" {
          }
        }
        n118 = property class="VI"(reference=w241, error in=w233) -> (reference out=w237:refnum<vi>, error out=w234:errorcluster, "VIType"=w240:T20)
        n119 = case shown="\"Control VI\"" w240 {
          tunnel: ["Control" ("pattern") "VI" ("pattern")] -> w239
          frame "Control VI" {
          }
          frame "Standard VI", Default {
          }
        }
        n120 = case shown="Default" w243 {
          selector: w243 -> [w280 _]
          tunnel: [w299 w414] -> w246
          tunnel: w242 -> [w298 w414]
          tunnel: w239 -> [w282 _]
          tunnel: w238 -> [w281 _]
          tunnel: w237 -> [w293 _]
          tunnel: w228 -> [w292 _]
          tunnel: w236 -> [w291 _]
          tunnel: w235 -> [w290 _]
          tunnel: w234 -> [w288 w413]
          tunnel: [w287 w413] -> w232
          tunnel: w231 -> [w286 _]
          tunnel: w227 -> [w285 _]
          tunnel: w224 -> [w279 _]
          frame Default {
            n121 = Build Path(base path=w292, name or relative path=w280) -> (appended path=w289:path)
            n122 = Format Into String(format string="This %s doesn't belong to a %s but there is a %s in this %s's %sfolder.\nDo you want to add this %s to the %s: %s?", w282, w281, w281, w282, w285, w282, w281, w280) -> (resulting string=w296:string)  [unwired: 2 in, 1 out]
            n123 = Format Into String(format string="Add %s to %s" ("T button name (\"OK\")"), w282, w281) -> (resulting string=w283:string)  [unwired: 2 in, 1 out]
            n124 = case shown="False" w279 {
              tunnel: w296 -> [w303 _]
              tunnel: "Ignore" ("F button name (\"Cancel\")") -> [w302 _]
              tunnel: [w301 _] -> w294
              tunnel: w283 -> [w300 _]
              frame False {
                n125 = Two Button Dialog(message=w303, 1:w302, 2:w300) -> (T button?=w301:bool)
              }
              frame True {
              }
            }
            n126 = case shown="True" w294 {
              tunnel: [w304 w316] -> w299
              tunnel: w298 -> [w304 w315]
              tunnel: w293 -> [_ _]
              tunnel: w291 -> [_ w314]
              tunnel: w290 -> [_ w313]
              tunnel: w289 -> [_ w312]
              tunnel: w288 -> [w305 w311]
              tunnel: [w305 w310] -> w287
              tunnel: w281 -> [_ w309]
              tunnel: [_ w307] -> _
              tunnel: w286 -> [_ w306]
              frame False {
              }
              frame True {
                n127 = case shown="\"class\", Default" w309 {
                  tunnel: w314 -> [w326 w360 w391]
                  tunnel: w313 -> [w319 w354 w386]
                  tunnel: w312 -> [w325 w359 w390]
                  tunnel: [w320 w355 w387] -> w308
                  tunnel: w311 -> [w324 w358 w389]
                  tunnel: [w323 w352 w384] -> w310
                  tunnel: w306 -> [w322 w357 w388]
                  frame "class", Default {
                    n128 = invoke class="App" method="LVClass.Open"(reference=w326, error in=w324, "Path"=w325) -> (error out=w321:errorcluster, "LVClass.Open"=w320:refnum<vi>)  [unwired: 1 in, 2 out]
                    n129 = case shown="Default" w322 {
                      selector: w322 -> [w337 _]
                      tunnel: w321 -> [w339 w349]
                      tunnel: w320 -> [w338 w350]
                      tunnel: w319 -> [w336 w346]
                      tunnel: [w335 w347] -> w318
                      tunnel: [w333 w348] -> w317
                      frame Default {
                        w341 = TRUE ("ExcludeDependencies")
                        n130 = invoke class="LVClassLibrary" method="Get All Descendents"(reference=w338, error in=w339, "Type"="Folder", "Exclude Dependencies"=w341, "ExcludeBuilds"=w341) -> (reference out=w329:refnum<vi>, error out=w334:errorcluster, "All Descendents"=w332:refnum<vi>[])  [unwired: 2 in, 4 out]
                        n131 = for {
                          tunnel: w332 -> [w345] mode=indexing
                          tunnel: [w343] -> w342 mode=indexing
                          n132 = property class="ProjectItem"(reference=w345) -> ("Name"=w344:string)  [unwired: 1 in, 2 out]
                          n133 = To Lower Case(string=w344) -> (all lower case string=w343:string)
                        }
                        n134 = Search 1D Array(1D array=w342, element=w337) -> (index of element=w331:i32)  [unwired: 1 in]
                        n135 = Less Than 0?(x=w331) -> (x < 0?=w330:bool)
                        n136 = Index Array(array=w332, index=w331) -> (element=w328:refnum<vi>)
                        n137 = Select(t=w329, s=w330, f=w328) -> (s? t:f=w327:refnum<vi>)
                        n138 = invoke class="ProjectItem" method="AddFile"(reference=w327, error in=w334, "Path"=w336) -> (error out=w333:errorcluster, "AddFile"=w335:refnum<vi>)  [unwired: 1 in, 2 out]
                        n139 = Close Reference(reference=w332, error in (no error)=w333) -> ()  [unwired: 1 out]
                      }
                      frame "" {
                        n140 = invoke class="LVClassLibrary" method="AddFile"(reference=w350, error in=w349, "Path"=w346) -> (error out=w348:errorcluster, "AddFile"=w347:refnum<vi>)  [unwired: 1 in, 2 out]
                      }
                    }
                    n141 = Close Reference(reference=w318, error in (no error)=w317) -> (error out=w323:errorcluster)
                  }
                  frame "library" {
                    n142 = invoke class="App" method="Library.Open"(reference=w360, error in=w358, "path"=w359) -> (error out=w356:errorcluster, "Open Library"=w355:refnum<vi>)  [unwired: 1 in, 2 out]
                    n143 = case shown="Default" w357 {
                      selector: w357 -> [w366 _]
                      tunnel: w356 -> [w368 w380]
                      tunnel: w355 -> [w367 w381]
                      tunnel: w354 -> [w365 w377]
                      tunnel: [w364 w378] -> w351
                      tunnel: [w362 w379] -> w353
                      frame Default {
                        w370 = TRUE ("ExcludeDependencies")
                        n144 = invoke class="Library" method="Get All Descendents"(reference=w367, error in=w368, "Type"="Folder", "Exclude Dependencies"=w370, "ExcludeBuilds"=w370) -> (error out=w363:errorcluster, "All Descendents"=w361:refnum<vi>[])  [unwired: 2 in, 5 out]
                        n145 = for {
                          tunnel: w361 -> [w376] mode=indexing
                          tunnel: [w374] -> w373 mode=indexing
                          n146 = property class="ProjectItem"(reference=w376) -> ("Name"=w375:string)  [unwired: 1 in, 2 out]
                          n147 = To Lower Case(string=w375) -> (all lower case string=w374:string)
                        }
                        n148 = Search 1D Array(1D array=w373, element=w366) -> (index of element=w371:i32)  [unwired: 1 in]
                        n149 = Index Array(array=w361, index=w371) -> (element=w372:refnum<vi>)
                        n150 = invoke class="ProjectItem" method="AddFile"(reference=w372, error in=w363, "Path"=w365) -> (error out=w362:errorcluster, "AddFile"=w364:refnum<vi>)  [unwired: 1 in, 2 out]
                        n151 = Close Reference(reference=w361, error in (no error)=w362) -> ()  [unwired: 1 out]
                      }
                      frame "" {
                        n152 = invoke class="Library" method="AddFile"(reference=w381, error in=w380, "Path"=w377) -> (error out=w379:errorcluster, "AddFile"=w378:refnum<vi>)  [unwired: 1 in, 2 out]
                      }
                    }
                    n153 = Close Reference(reference=w351, error in (no error)=w353) -> (error out=w352:errorcluster)
                  }
                  frame "X-control" {
                    n154 = invoke class="App" method="XControl.Open"(reference=w391, error in=w389, "Path"=w390) -> (error out=w382:errorcluster, "Open XControl"=w387:refnum<vi>)  [unwired: 1 in, 2 out]
                    n155 = case shown="Default" w388 {
                      selector: w388 -> [w397 _]
                      tunnel: w382 -> [w399 w411]
                      tunnel: w387 -> [w398 w412]
                      tunnel: w386 -> [w396 w408]
                      tunnel: [w395 w409] -> w383
                      tunnel: [w393 w410] -> w385
                      frame Default {
                        w401 = TRUE ("ExcludeDependencies")
                        n156 = invoke class="XCtlLib" method="Get All Descendents"(reference=w398, error in=w399, "Type"="Folder", "Exclude Dependencies"=w401, "ExcludeBuilds"=w401) -> (error out=w394:errorcluster, "All Descendents"=w392:refnum<vi>[])  [unwired: 2 in, 5 out]
                        n157 = for {
                          tunnel: w392 -> [w407] mode=indexing
                          tunnel: [w405] -> w404 mode=indexing
                          n158 = property class="ProjectItem"(reference=w407) -> ("Name"=w406:string)  [unwired: 1 in, 2 out]
                          n159 = To Lower Case(string=w406) -> (all lower case string=w405:string)
                        }
                        n160 = Search 1D Array(1D array=w404, element=w397) -> (index of element=w402:i32)  [unwired: 1 in]
                        n161 = Index Array(array=w392, index=w402) -> (element=w403:refnum<vi>)
                        n162 = invoke class="ProjectItem" method="AddFile"(reference=w403, error in=w394, "Path"=w396) -> (error out=w393:errorcluster, "AddFile"=w395:refnum<vi>)  [unwired: 1 in, 2 out]
                        n163 = Close Reference(reference=w392, error in (no error)=w393) -> ()  [unwired: 1 out]
                      }
                      frame "" {
                        n164 = invoke class="XCtlLib" method="AddFile"(reference=w412, error in=w411, "Path"=w408) -> (error out=w410:errorcluster, "AddFile"=w409:refnum<vi>)  [unwired: 1 in, 2 out]
                      }
                    }
                    n165 = Close Reference(reference=w383, error in (no error)=w385) -> (error out=w384:errorcluster)
                  }
                }
                n166 = Bundle By Name(cluster=w315, "LibraryRef"=w308) -> (w316:T6)
                n167 = invoke class="Library" method="Save"(reference=w308) -> (error out=w307:errorcluster)  [unwired: 3 in, 3 out]
              }
            }
          }
          frame "" {
          }
        }
      }
      frame "AnalyseFileName" {
        n168 = Unbundle By Name(w423) -> ("LibraryRef"=w421:refnum<vi>)
        n169 = Unbundle By Name(w423) -> ("Folder"=w429:path)
        n170 = local read "_VIPath"() -> (w425:path)
        n171 = Not A Number/Path/Refnum?(number/path/refnum=w429) -> (NaN/Path/Refnum?=w427:bool)
        n172 = Empty String/Path?(string/path=w429) -> (empty?=w428:bool)
        n173 = Not A Number/Path/Refnum?(number/path/refnum=w421) -> (NaN/Path/Refnum?=w422:bool)
        n174 = Or(x=w428, y=w427) -> (x .or. y?=w426:bool)
        n175 = case shown="False" w426 {
          tunnel: w423 -> [w453 w524]
          tunnel: [w452 w523] -> w431
          tunnel: [w451 w524] -> w430
          tunnel: w429 -> [w450 _]
          tunnel: w425 -> [w442 _]
          tunnel: w424 -> [w449 w523]
          tunnel: w422 -> [w448 _]
          tunnel: w421 -> [w447 _]
          tunnel: [w434 _] -> w419
          tunnel: w418 -> [w432 _]
          frame False {
            n176 = case shown="False" w448 {
              tunnel: [w489 w521] -> w452
              tunnel: w450 -> [w474 w517]
              tunnel: w442 -> [w475 w520]
              tunnel: [w480 w519] -> w445
              tunnel: [w487 w515] -> w446
              tunnel: [w463 w514] -> w433
              tunnel: w449 -> [w491 w518]
              tunnel: w447 -> [w492 _]
              tunnel: [w476 w516] -> w443
              tunnel: [w477 w513] -> w434
              frame False {
                n177 = property class="Library"(reference=w492, error in=w491) -> (error out=w489:errorcluster, "Name"=w486:string)  [unwired: 1 out]
                n178 = Strip Path(path=w475) -> (name=w488:string)  [unwired: 1 out]
                n179 = Match Pattern(string=w486, regular expression="\\2E[Ll][Vv][Ll][Ii][Bb]$") -> (before substring=w484:string)  [unwired: 1 in, 3 out]
                n180 = Match Pattern(string=w484, regular expression="\\2E[Ll][Vv][Cc][Ll][Aa][Ss][Ss]$") -> (before substring=w483:string, offset past match=w479:i32)  [unwired: 1 in, 2 out]
                n181 = Match Pattern(string=w483, regular expression="\\2E[Xx][Cc][Tt][Ll]$") -> (before substring=w482:string)  [unwired: 1 in, 3 out]
                n182 = call <resource>:"GDSIconEditor_FindPrefixInfo.vi"("_VIPath"=w475, "Folder"=w474) -> ("FolderFiles"=w470:path[], "Prefix"=w473:string, "Separator"=w472:string, "name"=w471:string, "FilePreFix+Separtor"=w468:string)  [unwired: 8 in, 1 out]
                n183 = Greater Or Equal To 0?(x=w479) -> (x >= 0?=w478:bool)
                n184 = case shown="True" w478 {
                  tunnel: w488 -> [_ w505]
                  tunnel: [w496 w502] -> w487
                  tunnel: [w495 w501] -> w469
                  tunnel: w482 -> [_ w500]
                  tunnel: [w497 w500] -> w480
                  tunnel: [w494 _] -> w477
                  tunnel: [w493 w499] -> w476
                  tunnel: w473 -> [w497 _]
                  tunnel: w472 -> [w496 _]
                  tunnel: w471 -> [w495 _]
                  tunnel: w468 -> [w494 _]
                  tunnel: w470 -> [w493 w499]
                  frame False {
                  }
                  frame True {
                    w502 = "[_\\s]+" ("Separator")
                    n185 = Concatenate Strings("^", w500, w502) -> (w512:string)
                    n186 = Match Pattern(string=w505, regular expression=w512) -> (before substring=w504:string, after substring=w503:string)  [unwired: 1 in, 2 out]
                    n187 = Concatenate Strings(w504, w503) -> (w498:string)
                    n188 = Match Pattern(string=w498, regular expression="\\2Evi$") -> (before substring=w508:string)  [unwired: 1 in, 3 out]
                    n189 = Match Pattern(string=w508, regular expression="\\2Ectl$") -> (before substring=w509:string)  [unwired: 1 in, 3 out]
                    n190 = Match Pattern(string=w509, regular expression="\\2Evi[mt]$") -> (before substring=w501:string)  [unwired: 1 in, 3 out]
                  }
                }
                n191 = Concatenate Strings("$" ("string"), w468) -> (w466:string)
                n192 = Match Pattern(string=w469, regular expression=w466) -> (before substring=w465:string, after substring=w464:string)  [unwired: 1 in, 2 out]
                n193 = Concatenate Strings(w465, w464) -> (w463:string)
              }
              frame True {
                n194 = call <resource>:"GDSIconEditor_FindPrefixInfo.vi"("_VIPath"=w520, "Folder"=w517, "error in (no error)"=w518) -> ("FolderFiles"=w516:path[], "Prefix"=w519:string, "Separator"=w515:string, "name"=w514:string, "FilePreFix+Separtor"=w513:string, "error out"=w521:errorcluster)  [unwired: 7 in]
              }
            }
            n195 = for {
              tunnel: w443 -> [w455] mode=indexing
              shift-right: [w457] -> w441
              shift-left: path[] [] -> [w458]
              tunnel: w442 -> [w454]
              n196 = Not Equal?(x=w455, y=w454) -> (x != y?=w456:bool)
              n197 = case shown="True" w456 {
                tunnel: w458 -> [w459 w462]
                tunnel: [w459 w461] -> w457
                tunnel: w455 -> [_ w460]
                frame False {
                }
                frame True {
                  n198 = Build Array (concatenate)(w462, w460) -> (w461:path[])
                }
              }
            }
            n199 = Array Size(array=w441) -> (size(s)=w439:i32)
            n200 = Greater Than 0?(x=w439) -> (x > 0?=w438:bool)
            n201 = Select(t=u8 0, s=w438, f=u8 2 ("Disabled")) -> (s? t:f=w440:u8)
            n202 = property on="_ApplyHeaderToAll" class="Bool (strict)"("Disabled"=w440) -> ()  [unwired: 2 in, 2 out]
            n203 = call <resource>:"GDSIconEditor_SplitNameInRows.vi"("FileNameFilter"=w432, "name"=w433) -> ("result string"=w435:string)  [unwired: 9 in]
            n204 = Bundle By Name(cluster=w453, "VIs"=w441, "Prefix"=w445, "Separator"=w446, "StartMethodName"=w435) -> (w451:T6)
          }
          frame True {
            n205 = local write "_MethodIconName"("NoFilePath" ("Method Icon Name")) -> ()
          }
        }
        "_FilePrefixFound" <- w419
      }
      frame "Auto find header" {
        n206 = Unbundle By Name(w536) -> ("AppRef"=w534:refnum<vi>, "Scope"=w535:T3, "VIs"=w533:path[])
        n207 = Unbundle By Name(w536) -> ("ViRef"=w526:refnum<vi>)
        n208 = Unbundle By Name(w536) -> ("LibraryRef"=w537:refnum<vi>)
        n209 = To Variant(anything=w526) -> (Variant=w525:variant)
        n210 = for {
          tunnel: w533 -> [w542] mode=indexing
          tunnel: [w541] -> w532 mode=indexing
          n211 = To Variant(anything=w542) -> (Variant=w541:variant)
        }
        n212 = Build Array (concatenate)(w525, w532, w525) -> (w531:variant[])
        n213 = Not A Number/Path/Refnum?(number/path/refnum=w537) -> (NaN/Path/Refnum?=w538:bool)
        n214 = case shown="True" w538 {
          tunnel: [w548 w710] -> w529
          tunnel: [w547 w704] -> w540
          tunnel: w531 -> [_ w708]
          tunnel: w539 -> [w546 w705]
          tunnel: w536 -> [w552 w711]
          tunnel: w537 -> [w545 _]
          tunnel: w535 -> [w550 _]
          tunnel: w534 -> [_ _]
          tunnel: w527 -> [w544 w691]
          tunnel: w525 -> [w543 _]
          frame False {
            n215 = Bundle By Name(cluster=w552, "Header exists"=TRUE) -> (w549:T6)
            n216 = case shown="No Error" w546 {
              selector: w546 -> [w597 _]
              tunnel: w545 -> [w596 _]
              tunnel: w550 -> [w604 _]
              tunnel: w549 -> [w595 w672]
              tunnel: [w594 w671] -> w548
              tunnel: [w591 w667] -> w547
              tunnel: w545 -> [_ w648]
              tunnel: w546 -> [_ w646]
              tunnel: w544 -> [w561 _]
              tunnel: w543 -> [w554 _]
              frame No Error {
                w602 = u8 32 ("x")
                w571 = u32 0
                n217 = call <resource>:"GDSLvClass_ReadClassColors.vi"("Library Refnum"=w596, "error in (no error)"=w597) -> ("Library Refnum"=w583:refnum<vi>, "LvClassIconSettings"=w555:T21, "LvClassIconSettingsFound"=w577:bool, "error out"=w590:errorcluster)  [unwired: 12 in, 2 out]
                n218 = Unbundle By Name(w555) -> ("ColorPrivate"=w574:u32, "ColorProtected"=w575:u32, "ColorPublic"=w576:u32, "Frame"=w573:u32, "Body Text"=w572:u32, "Frame thickness"=w559:u8, "ClassBodyIcon"=w557:string)
                n219 = To Variant(anything=w583) -> (Variant=w553:variant)
                n220 = case shown="\"Private\"" w604 {
                  tunnel: [w642 w643 w644] -> w589
                  tunnel: w576 -> [w642 _ _]
                  tunnel: w575 -> [_ w643 _]
                  tunnel: w574 -> [_ _ w644]
                  frame "Public", Default {
                  }
                  frame "Proteced" {
                  }
                  frame "Private" {
                  }
                }
                n221 = Build Array(w553, w554) -> (w556:variant[])
                n222 = for {
                  tunnel: [w614] -> w586
                  tunnel: [w613] -> w585
                  tunnel: [w612] -> w584
                  tunnel: w556 -> [w611] mode=indexing
                  tunnel: [w610] -> w564
                  tunnel: [w609] -> w563
                  tunnel: [w608] -> w562
                  tunnel: [w607] -> w560
                  tunnel: [w606] -> w558
                  shift-right: [w616] -> w591
                  shift-left: w590 -> [w615]
                  stop <- w605 stop-if-true
                  n223 = call <resource>:"GDSLvIcon_AnalyseViIcon.vi"("ViRef/LvCLassRef/LvLibRef/ViPath/2D_Image"=w611, "error in (no error)"=w615) -> ("BodyTextColor"=w612:u32, "Splitter0px"=w607:bool, "FrameColor"=w614:u32, "FrameThickness(1)"=w606:u32, "ValidHeaderIcon"=w605:bool, "DefaultIcon"=w608:bool, "HeaderIcon"=w610:u8[][], "HeaderBkColor"=w609:u32, "BodyBkColor"=w613:u32, "error out"=w616:errorcluster)  [unwired: 4 in, 4 out]
                }
                n224 = case shown="False" w577 {
                  tunnel: [w624 w641] -> w570
                  tunnel: w589 -> [_ w641]
                  tunnel: [w622 w640] -> w581
                  tunnel: w572 -> [_ w640]
                  tunnel: [w627 w639] -> w588
                  tunnel: w573 -> [_ w639]
                  tunnel: [w628 w638] -> w587
                  tunnel: w559 -> [_ w638]
                  tunnel: w558 -> [w628 _]
                  tunnel: w586 -> [w627 _]
                  tunnel: w585 -> [w625 _]
                  tunnel: w584 -> [w623 _]
                  tunnel: w562 -> [w626 _]
                  tunnel: w561 -> [w621 _]
                  frame False {
                    n225 = case shown="False" w626 {
                      tunnel: w625 -> [w630 _]
                      tunnel: [w630 w632] -> w624
                      tunnel: [w629 u32 0] -> w622
                      tunnel: w623 -> [w629 _]
                      tunnel: w621 -> [_ w631]
                      frame False {
                      }
                      frame True {
                        n226 = Array Size(array=w631) -> (size(s)=w633:i32)
                        n227 = Random Number (0-1)() -> (number: 0 to 1=w635:dbl)
                        n228 = Multiply(x=w633, y=w635) -> (x*y=w636:dbl)
                        n229 = Round Toward -Infinity(1:w636) -> (0:w634:dbl)
                        n230 = Index Array(array=w631, index=w634) -> (element=w632:u32)
                      }
                    }
                  }
                  frame True {
                  }
                }
                n231 = case shown="True" w560 {
                  tunnel: [w619 w620] -> w600
                  tunnel: w558 -> [w617 w620]
                  frame False {
                    n232 = Multiply(x=w617, y=u8 2) -> (x*y=w619:u32)
                  }
                  frame True {
                  }
                }
                n233 = Array Size(array=w564) -> (size(s)=w598:i32[])
                n234 = local read "_BackgroundColor"() -> (w568:T2)
                n235 = Index Array(array=w598) -> (element #1=w599:i32)  [unwired: 2 in, 1 out]
                n236 = Equal?(x=w570, y=w581) -> (x = y?=w582:bool)
                n237 = Bundle(cluster=w568, "Color"=w570) -> (w569:T2)  [unwired: 1 in]
                n238 = Add(x=w599, y=w600) -> (x+y=w601:u32)
                n239 = Equal?(x=w570, y=w571) -> (x = y?=w580:bool)
                n240 = Increment(x=w601) -> (x+1=w603:u32)
                n241 = local write "_BackgroundColor"(w569) -> ()
                n242 = local read "_BodyTextColor"() -> (w565:T2)
                n243 = Select(t=u32 16777215, s=w580, f=w571) -> (s? t:f=w578:u32)
                n244 = Subtract(x=w602, y=w603) -> (x-y=w593:u32)
                n245 = Subtract(x=w602, y=w600) -> (x-y=w592:u32)
                n246 = Bundle By Name(cluster=w595, "FrameColor"=w588, "Frame thickness"=w587, "HeaderIcon"=w564, "HeaderBkColor"=w563, "BodyIconHeight"=w593, "BodyIconWidth"=w592, "ClassBodyIcon"=w557, "Splitter0px"=w560) -> (w594:T6)
                n247 = Select(t=w578, s=w582, f=w581) -> (s? t:f=w567:u32)
                n248 = Bundle(cluster=w565, "Color"=w567) -> (w566:T2)  [unwired: 1 in]
                n249 = local write "_BodyTextColor"(w566) -> ()
              }
              frame Error {
                w652 = refnum<vi> refnum  # Library
                w677 = u8 32 ("x")
                w660 = u32 0
                n250 = To More Specific Class(target class=w652, reference=w648, error in=w646) -> (specific class reference=w649:refnum<vi>, error out=w651:errorcluster)
                n251 = case shown="Error" w651 {
                  selector: w651 -> [w683 _]
                  tunnel: [w684 w687] -> w650
                  tunnel: w649 -> [w684 _]
                  tunnel: w648 -> [_ w688]
                  tunnel: [w683 w686] -> w647
                  tunnel: w646 -> [_ w685]
                  frame No Error {
                  }
                  frame Error {
                    w689 = refnum<vi> refnum  # XControlLibrary
                    n252 = To More Specific Class(target class=w689, reference=w688, error in=w685) -> (specific class reference=w687:refnum<vi>, error out=w686:errorcluster)
                  }
                }
                n253 = call <resource>:"GDSLvIcon_AnalyseViIcon.vi"("ViRef/LvCLassRef/LvLibRef/ViPath/2D_Image"=w650, "error in (no error)"=w647) -> ("BodyTextColor"=w653:u32, "Splitter0px"=w645:bool, "FrameColor"=w666:u32, "FrameThickness(1)"=w665:u32, "HeaderIcon"=w670:u8[][], "BodyBkColor"=w654:u32, "error out"=w667:errorcluster)  [unwired: 4 in, 7 out]
                n254 = case shown="True" w645 {
                  tunnel: [w681 w682] -> w675
                  tunnel: w665 -> [w679 w682]
                  frame False {
                    n255 = Multiply(x=w679, y=u8 2) -> (x*y=w681:u32)
                  }
                  frame True {
                  }
                }
                n256 = Array Size(array=w670) -> (size(s)=w673:i32[])
                n257 = local read "_BackgroundColor"() -> (w658:T2)
                n258 = Equal?(x=w654, y=w653) -> (x = y?=w664:bool)
                n259 = Index Array(array=w673) -> (element #1=w674:i32)  [unwired: 2 in, 1 out]
                n260 = Bundle(cluster=w658, "Color"=w654) -> (w659:T2)  [unwired: 1 in]
                n261 = Add(x=w674, y=w675) -> (x+y=w676:u32)
                n262 = local write "_BackgroundColor"(w659) -> ()
                n263 = Equal?(x=w654, y=w660) -> (x = y?=w663:bool)
                n264 = Increment(x=w676) -> (x+1=w678:u32)
                n265 = Select(t=u32 16777215, s=w663, f=w660) -> (s? t:f=w661:u32)
                n266 = local read "_BodyTextColor"() -> (w655:T2)
                n267 = Select(t=w661, s=w664, f=w653) -> (s? t:f=w657:u32)
                n268 = Subtract(x=w677, y=w678) -> (x-y=w669:u32)
                n269 = Subtract(x=w677, y=w675) -> (x-y=w668:u32)
                n270 = Bundle(cluster=w655, "Color"=w657) -> (w656:T2)  [unwired: 1 in]
                n271 = local write "_BodyTextColor"(w656) -> ()
                n272 = Bundle By Name(cluster=w672, "FrameColor"=w666, "Frame thickness"=w665, "HeaderIcon"=w670, "BodyIconHeight"=w669, "BodyIconWidth"=w668, "Splitter0px"=w645) -> (w671:T6)
              }
            }
          }
          frame True {
            w720 = u8 32 ("x")
            n273 = for {
              tunnel: [w757] -> w718
              tunnel: [w756] -> w698
              tunnel: w708 -> [w755] mode=indexing
              tunnel: [w754] -> w707
              tunnel: [w753] -> w706
              tunnel: [w752] -> w695
              tunnel: w705 -> [w751]
              tunnel: [w750] -> w704
              tunnel: [w749] -> w693
              tunnel: [w748] -> w694
              tunnel: [w747] -> w692
              tunnel: [w746] -> w690
              stop <- w749 stop-if-true
              n274 = call <resource>:"GDSLvIcon_AnalyseViIcon.vi"("ViRef/LvCLassRef/LvLibRef/ViPath/2D_Image"=w755, "error in (no error)"=w751) -> ("BodyTextColor"=w752:u32, "Splitter0px"=w746:bool, "FrameColor"=w753:u32, "FrameThickness(1)"=w754:u32, "ValidHeaderIcon"=w749:bool, "DefaultIcon"=w747:bool, "HeaderIcon"=w757:u8[][], "HeaderBkColor"=w748:u32, "BodyBkColor"=w756:u32, "error out"=w750:errorcluster)  [unwired: 4 in, 4 out]
            }
            n275 = case shown="False" w692 {
              tunnel: w698 -> [w730 _]
              tunnel: [w729 w741] -> w697
              tunnel: [w728 u32 0] -> w696
              tunnel: w695 -> [w726 _]
              tunnel: w691 -> [_ w739]
              frame False {
                n276 = Equal?(x=w730, y=w726) -> (x = y?=w731:bool)
                n277 = Equal?(x=w726, y=u32 0) -> (x = y?=w727:bool)
                n278 = case shown="True" w731 {
                  tunnel: w726 -> [w732 _]
                  tunnel: w730 -> [w733 w738]
                  tunnel: [w733 w738] -> w729
                  tunnel: [w732 w736] -> w728
                  tunnel: w727 -> [_ w737]
                  frame False {
                  }
                  frame True {
                    n279 = Select(t=u32 16777215, s=w737, f=u32 0) -> (s? t:f=w736:u32)
                  }
                }
              }
              frame True {
                n280 = Array Size(array=w739) -> (size(s)=w742:i32)
                n281 = Random Number (0-1)() -> (number: 0 to 1=w744:dbl)
                n282 = Multiply(x=w742, y=w744) -> (x*y=w745:dbl)
                n283 = Round Toward -Infinity(1:w745) -> (0:w743:dbl)
                n284 = Index Array(array=w739, index=w743) -> (element=w741:u32)
              }
            }
            n285 = Array Size(array=w718) -> (size(s)=w719:i32[])
            n286 = case shown="True" w690 {
              tunnel: [w722 w724] -> w709
              tunnel: w707 -> [w721 w724]
              frame False {
                n287 = Multiply(x=w721, y=u8 2) -> (x*y=w722:u32)
              }
              frame True {
              }
            }
            n288 = Index Array(array=w719) -> (element #1=w703:i32)  [unwired: 2 in, 1 out]
            n289 = local read "_BodyTextColor"() -> (w712:T2)
            n290 = Equal To 0?(x=w703) -> (x = 0?=w702:bool)
            n291 = local read "_BackgroundColor"() -> (w715:T2)
            n292 = Add(x=w703, y=w709) -> (x+y=w700:u32)
            n293 = Bundle(cluster=w715, "Color"=w697) -> (w714:T2)  [unwired: 1 in]
            n294 = Increment(x=w700) -> (x+1=w701:u32)
            n295 = local write "_BackgroundColor"(w714) -> ()
            n296 = Select(t=w700, s=w702, f=w701) -> (s? t:f=w699:u32)
            n297 = Bundle(cluster=w712, "Color"=w696) -> (w713:T2)  [unwired: 1 in]
            n298 = Subtract(x=w720, y=w699) -> (x-y=w717:u32)
            n299 = Subtract(x=w720, y=w709) -> (x-y=w716:u32)
            n300 = local write "_BodyTextColor"(w713) -> ()
            n301 = Bundle By Name(cluster=w711, "FrameColor"=w706, "Frame thickness"=w707, "HeaderIcon"=w718, "BodyIconHeight"=w717, "BodyIconWidth"=w716, "Header exists"=w693, "HeaderBkColor"=w694, "Splitter0px"=w690) -> (w710:T6)
          }
        }
        n302 = Unbundle By Name(w529) -> ("Header exists"=w528:bool)
        n303 = property on="_HideHeader" class="Bool (strict)"("Visible"=w528) -> ()  [unwired: 2 in, 2 out]
      }
      frame "UseBeforePicture" {
        (unwired) "UpdateIcon"
        w777 = u32 0
        w789 = u8 32 ("x")
        (unwired) "DoIconTextOCR"
        n304 = Unbundle By Name(w791) -> ("ViRef"=w769:refnum<vi>)
        n305 = call <resource>:"GDSLvIcon_AnalyseViIcon.vi"("ViRef/LvCLassRef/LvLibRef/ViPath/2D_Image"=w769, "error in (no error)"=w767) -> ("BodyTextColor"=w763:u32, "Splitter0px"=w758:bool, "FrameColor"=w782:u32, "FrameThickness(1)"=w768:u32, "DefaultIcon"=w764:bool, "HeaderIcon"=w771:u8[][], "HeaderBkColor"=w770:u32, "BodyIcon"=w766:u8[][], "BodyBkColor"=w762:u32, "error out"=w792:errorcluster)  [unwired: 4 in, 4 out]
        n306 = case shown="True" w764 {
          tunnel: w762 -> [w799 _]
          tunnel: [w799 w801] -> w759
          tunnel: [w798 u32 0] -> w761
          tunnel: w763 -> [w798 _]
          tunnel: w760 -> [_ w800]
          frame False {
          }
          frame True {
            n307 = Array Size(array=w800) -> (size(s)=w802:i32)
            n308 = Random Number (0-1)() -> (number: 0 to 1=w804:dbl)
            n309 = Multiply(x=w802, y=w804) -> (x*y=w805:dbl)
            n310 = Round Toward -Infinity(1:w805) -> (0:w803:dbl)
            n311 = Index Array(array=w800, index=w803) -> (element=w801:u32)
          }
        }
        n312 = Array Size(array=w771) -> (size(s)=w785:i32[])
        n313 = case shown="True" w758 {
          tunnel: [w796 w797] -> w787
          tunnel: w768 -> [w794 w797]
          frame False {
            n314 = Multiply(x=w794, y=u8 2) -> (x*y=w796:u32)
          }
          frame True {
          }
        }
        n315 = local read "_BackgroundColor"() -> (w775:T2)
        n316 = Equal?(x=w759, y=w761) -> (x = y?=w781:bool)
        n317 = Bundle(cluster=w775, "Color"=w759) -> (w776:T2)  [unwired: 1 in]
        n318 = Index Array(array=w785) -> (element #1=w786:i32)  [unwired: 2 in, 1 out]
        n319 = local write "_BackgroundColor"(w776) -> ()
        n320 = Add(x=w786, y=w787) -> (x+y=w788:u32)
        n321 = Increment(x=w788) -> (x+1=w790:u32)
        n322 = Equal?(x=w759, y=w777) -> (x = y?=w780:bool)
        n323 = Select(t=u32 16777215, s=w780, f=w777) -> (s? t:f=w778:u32)
        n324 = Subtract(x=w789, y=w790) -> (x-y=w784:u32)
        n325 = Subtract(x=w789, y=w787) -> (x-y=w783:u32)
        n326 = Select(t=w778, s=w781, f=w761) -> (s? t:f=w774:u32)
        n327 = local read "_BodyTextColor"() -> (w772:T2)
        n328 = Bundle(cluster=w772, "Color"=w774) -> (w773:T2)  [unwired: 1 in]
        n329 = Bundle By Name(cluster=w791, "FrameColor"=w782, "Frame thickness"=w768, "HeaderIcon"=w771, "HeaderBkColor"=w770, "BodyIcon"=w766, "BodyIconHeight"=w784, "BodyIconWidth"=w783, "Splitter0px"=w758) -> (w793:T6)
        n330 = local write "_BodyTextColor"(w773) -> ()
      }
      frame "DoIconTextOCR", "DoIconTextOCR_Before" {
        # "First Time and OCR Text Found"
        n331 = Unbundle By Name(w817) -> ("FirstTime"=w810:bool, "StartMethodName"=w818:string, "ViRef"=w826:refnum<vi>)
        n332 = call <resource>:"GDSLvIcon_AnalyseViIcon.vi"("ViRef/LvCLassRef/LvLibRef/ViPath/2D_Image"=w826, "DoATextOCR(False)"=TRUE, "error in (no error)"=w828) -> ("BodyText(OCR)"=w813:string, "error out"=w829:errorcluster)  [unwired: 3 in, 12 out]
        n333 = call <resource>:"GOOP_OCREvaluation.vi"("OcrText"=w813, "Viname"=w818) -> ("Match"=w808:bool)  [unwired: 9 in]
        n334 = Not Equal?(x=w824, y="DoIconTextOCR_Before") -> (x != y?=w822:bool)
        n335 = Empty String/Path?(string/path=w813) -> (empty?=w812:bool)
        n336 = Compound Arithmetic op=AND(w810, invert w812) -> (w814:bool)
        n337 = local read "_OCR"() -> (w807:bool)
        n338 = And(x=w810, y=w808) -> (x .and. y?=w809:bool)
        n339 = Or(x=w809, y=w807) -> (x .or. y?=w811:bool)
        n340 = Select(t=w813, s=w811, f=w818) -> (s? t:f=w825:string)
        n341 = case shown="True" w814 {
          tunnel: w808 -> [_ w830]
          frame False {
          }
          frame True {
            w831 = FALSE ("Boolean Text.Font:Bold")
            n342 = property on="_OCR" class="Bool (strict)"("BoolText.FontBold"=w831, "BoolText.FontUnder"=w831, "Visible"=TRUE, "Value"=w830) -> ()  [unwired: 2 in, 2 out]
          }
        }
        n343 = local write "_MethodIconName"(w825) -> ()
        n344 = Bundle By Name(cluster=w817, "FirstTime"=FALSE) -> (w816:T6)
        n345 = Select(t="GuessIconSize", s=w822, f="UpdateIcon,ShowLayoutChange") -> (s? t:f=w819:string)
      }
      frame "GuessIconSize" {
        n346 = Unbundle By Name(w841) -> ("ViRef"=w835:refnum<vi>)
        n347 = property class="VI"(reference=w835) -> ("VIType"=w834:T20)  [unwired: 1 in, 2 out]
        n348 = case shown="Default" w834 {
          tunnel: w843 -> [w848 w863]
          tunnel: [w848 w862] -> w842
          tunnel: [0 ("StartRow") w860] -> w839
          tunnel: [w849 w859] -> w838
          tunnel: [i32[] [] ("ConnectorPaneHeight") w858] -> w837
          tunnel: [TRUE FALSE] -> w836
          tunnel: w835 -> [_ w852]
          tunnel: [_ TRUE] -> w833
          frame "Control VI", "Polymorphic VI" {
            w849 = u16 0 items=["Full", "1 c-term high", "2 c-term high", "3 c-term high"] ("_IconSize")
          }
          frame Default {
            n349 = call <resource>:"GOOP_GetControlRearrangement.vi"("VI Refnum"=w852, "_IconSize"=IconSize."Full" ("NewIconSize"), "error in (no error)"=w863) -> ("StartRow"=w860:i32, "ControlsToMove"=w854:T22, "ConnectorPaneHeight"=w858:i32[], "NumberOfTerminalAtStart"=w856:i32, "error out"=w862:errorcluster)  [unwired: 10 in, 2 out]
            n350 = Array Size(array=w854) -> (size(s)=w853:i32)
            n351 = Equal To 0?(x=w853) -> ()  [unwired: 1 out]
            n352 = Array Size(array=w858) -> (size(s)=w857:i32)
            n353 = Equal?(x=w857, y=w856) -> (x = y?=w855:bool)
            n354 = case shown="True" w855 {
              tunnel: [w865 w870] -> w859
              tunnel: w856 -> [w864 _]
              frame False {
                n355 = case shown="3" w864 {
                  tunnel: [w866 w867 w868 w869] -> w865
                  frame 1 {
                    w866 = u16 1 items=["Full", "1 c-term high", "2 c-term high", "3 c-term high"] ("_IconSize")
                  }
                  frame 2 {
                    w867 = u16 2 items=["Full", "1 c-term high", "2 c-term high", "3 c-term high"] ("_IconSize")
                  }
                  frame 3 {
                    w868 = u16 3 items=["Full", "1 c-term high", "2 c-term high", "3 c-term high"] ("_IconSize")
                  }
                  frame Default {
                    w869 = u16 0 items=["Full", "1 c-term high", "2 c-term high", "3 c-term high"] ("_IconSize")
                  }
                }
              }
              frame True {
                w870 = u16 0 items=["Full", "1 c-term high", "2 c-term high", "3 c-term high"] ("_IconSize")
              }
            }
          }
        }
        n356 = property on="_IconSize" class="Ring (strict)"("Visible"=w833) -> ()  [unwired: 2 in, 2 out]
        n357 = local write "_IconSize"(w838) -> ()
        n358 = Bundle By Name(cluster=w841, "StartRow"=w839, "NoControlsToMove"=w836, "ConnectorPaneHeight"=w837, "StartIconSize"=w838) -> (w840:T6)
      }
      frame "Generate icon" {
        n359 = Unbundle By Name(w874) -> ("Scope"=w875:T3)  [unwired: 1 out]
        n360 = case shown="True" TRUE {
          tunnel: w877 -> [w878 w935]
          tunnel: [w878 w934] -> w876
          tunnel: w875 -> [_ _]
          tunnel: w874 -> [w879 w905]
          tunnel: [w879 w931] -> w873
          frame False {
          }
          frame True {
            n361 = Unbundle By Name(w905) -> ("StartIconSize"=w912:u16, "StartRow"=w908:i32, "FrameColor"=w913:u32, "Frame thickness"=w924:i32, "HeaderIcon"=w917:u8[][])
            n362 = local read "_MethodIconName"() -> (w932:string)
            n363 = local read "_FontCapitalOnly"() -> (w933:bool)
            n364 = local read "_FontCompression"() -> (w920:enum16{"Auto", "On", "Off"})
            n365 = local read "_BackgroundColor"() -> (w930:T2)
            n366 = Unbundle By Name(w905) -> ("Frame thickness"=w896:i32, "ConnectorPaneHeight"=w919:i32[], "BodyIconHeight"=w918:i32, "BodyIconWidth"=w915:i32, "Splitter0px"=w880:bool)
            n367 = local read "_TextAlignment"() -> (w906:u16)
            n368 = local read "_HideHeader"() -> (w882:bool)
            n369 = local read "_IconSize"() -> (w911:u16)
            n370 = local read "_BodyTextColor"() -> (w928:T2)
            n371 = Unbundle By Name(w928) -> ("Color"=w895:u32)
            n372 = Unbundle By Name(w930) -> ("Color"=w929:u32)
            n373 = Not Equal?(x=w912, y=w911) -> (x != y?=w910:bool)
            n374 = Compound Arithmetic op=AND(invert w882, w880) -> (w881:bool)
            n375 = Select(t=0, s=w910, f=w908) -> (s? t:f=w885:i32)
            n376 = call <resource>:"GDSIconEditor_IconSizeAdjustment.vi"("BodyIconHeightIn"=w918, "HideHeader"=w882, "ConnectorPaneHeight"=w919, "Frame thickness"=w896, "_IconSize"=w911, "HeaderIconIn"=w917) -> ("HeaderIconOut"=w916:u8[][], "BodyIconHeightOut"=w914:u32, "ImageRows"=w883:i32)  [unwired: 3 in]
            n377 = Unbundle By Name(w905) -> ("OldOffset.X"=w902:i32, "OldOffset.Y"=w898:i32, "CurrentIcon"=w892:T13)
            n378 = Unbundle By Name(w905) -> ("Offset"=w901:cluster{"X":i32, "Y":i32})
            n379 = Bundle By Name(cluster=T10 {"Text"="", "Allow Only Capital Chars"=FALSE, "Compression"=enum."Auto", "Alignment"=enum."Center"} ("IconTextDataType"), "Text"=w932, "Allow Only Capital Chars"=w933, "Compression"=w920, "Alignment"=w906) -> (w926:T10)
            n380 = Unbundle By Name(w901) -> ("X"=w900:i32, "Y"=w897:i32)
            n381 = call <resource>:"GDSLvIcon_GenerateIconText.vi"("Text"=w926, "TextPixelHeight(5-30)"=w914, "Foreground color"=w895, "Background color"=w929, "error in (no error)"=w935, "Offset"=w901, "Text Pixel width(32-FrameThicknes*2))"=w915) -> ("X-Limited"=w904:bool, "Y-Limited"=w899:bool, "TextOut"=w893:u8[][], "TextBounds"=w891:T23, "error out"=w925:errorcluster)  [unwired: 8 in]
            n382 = call <resource>:"GDSLvIcon_CreateIconPicture.vi"("FrameColor"=w913, "FrameThickness(1)"=w924, "HeaderIconIn"=w916, "BodyIconIn"=w893, "error in (no error)"=w925, "ImageRows(32)"=w883, "BigSizeIcon(x6)"=4, "RowStart(0)"=w885, "BgIcon"=w892, "0px Splitter(False)"=w881) -> ("WholeIconOut"=w922:u8[][], "IconPictureOut"=→"_After":picture, "LargeIconPictureOut(x6)"=→"_IconPreview":picture, "BodyOffset"=w889:cluster{"X":i32, "Y":i32}, "error out"=w934:errorcluster)  [unwired: 4 in, 1 out]
            n383 = Unbundle(w889) -> ("X"=w886:i32, "Y"=w887:i32)
            n384 = Bundle("Y"=w887, "X"=w886, "Y"=w887, "X"=w886) -> (w888:cluster{"Y":i32, "X":i32, "Y":i32, "X":i32})  [unwired: 1 in]
            n385 = Add(x=w888, y=w891) -> (x+y=w890:cluster{i32, i32, i32, i32})
            n386 = Select(t=w902, s=w904, f=w900) -> (s? t:f=w903:i32)
            n387 = Select(t=w898, s=w899, f=w897) -> (s? t:f=w884:i32)
            n388 = Bundle By Name(cluster=w905, "Offset.X"=w903, "Offset.Y"=w884, "Icon exist"=TRUE, "IconOut"=w922, "BodyIcon"=w893, "TextBounds"=w890, "RowStart(0)"=w885, "ImageRows(32)"=w883) -> (w931:T6)
          }
        }
      }
      frame "UpdateIcon", "UpdateIcon,ShowLayoutChange" {
        # "ImageRows"
        n389 = Unbundle By Name(w961) -> ("Frame thickness"=w942:i32, "ConnectorPaneHeight"=w941:i32[], "BodyIconHeight"=w940:i32, "BodyIcon"=w962:u8[][], "Splitter0px"=w936:bool)
        n390 = Unbundle By Name(w961) -> ("StartIconSize"=w969:u16, "StartRow"=w966:i32, "FrameColor"=w970:u32, "Frame thickness"=w974:i32, "HeaderIcon"=w944:u8[][])
        n391 = disable-structure shown="Enabled" {
          disable-tunnel: w961 -> [w978 w997]
          disable-tunnel: [w977 w995] -> w959
          frame Disabled {
            w988 = T13 {"BgIcon"=[], "BgIconOffset"={"X"=0, "Y"=0}, "BgIconMask"=[], "ColorsOkayforiconToBeOnTopOf"=[]}  # BgIcon
            n392 = local read "_BackgroundColor"() -> (w985:T2)
            n393 = Unbundle By Name(w985) -> ("Color"=w980:u32)
            n394 = Unbundle By Name(w978) -> ("BgIcon"=w987:u8[][], "BgIconOffset"=w986:cluster{"X":i32, "Y":i32}, "BgIconMask"=w983:u8[], "HeaderBkColor"=w982:u32)
            n395 = call <resource>:"GDSLvIcon_Convert24bitTo8bitColor.vi"("Color 24bit In"=w982) -> ("Color out(256)"=w981:u8)  [unwired: 15 in, 3 out]
            n396 = call <resource>:"GDSLvIcon_Convert24bitTo8bitColor.vi"("Color 24bit In"=w980) -> ("Color out(256)"=w979:u8)  [unwired: 15 in, 3 out]
            n397 = Build Array(w981, w979) -> (w984:u8[])
            n398 = Bundle By Name(cluster=w988, "BgIcon"=w987, "BgIconOffset"=w986, "BgIconMask"=w983, "ColorsOkayforiconToBeOnTopOf"=w984) -> (w977:T13)
          }
          frame Enabled {
            n399 = Unbundle By Name(w997) -> ("CurrentIcon"=w996:T13, "HeaderBkColor"=w990:u32)
            n400 = local read "_BackgroundColor"() -> (w994:T2)
            n401 = Unbundle By Name(w994) -> ("Color"=w993:u32)
            n402 = call <resource>:"GDSLvIcon_Convert24bitTo8bitColor.vi"("Color 24bit In"=w990) -> ("Color out(256)"=w989:u8)  [unwired: 15 in, 3 out]
            n403 = call <resource>:"GDSLvIcon_Convert24bitTo8bitColor.vi"("Color 24bit In"=w993) -> ("Color out(256)"=w992:u8)  [unwired: 15 in, 3 out]
            n404 = Build Array(w989, w992) -> (w991:u8[])
            n405 = Bundle By Name(cluster=w996, "ColorsOkayforiconToBeOnTopOf"=w991) -> (w995:T13)
          }
        }
        n406 = local read "_IconSize"() -> (w943:u16)
        n407 = case shown="Default" w943 {
          tunnel: w944 -> [w1019 _]
          tunnel: [w1019 _] -> w945
          frame Default {
          }
          frame 1 {
          }
        }
        n408 = Not Equal?(x=w969, y=w943) -> (x != y?=w968:bool)
        n409 = Array Size(array=w945) -> (size(s)=w972:i32[])
        n410 = Index Array(array=w972) -> (element=w971:i32)  [unwired: 1 in]
        n411 = Select(t=0, s=w968, f=w966) -> (s? t:f=w947:i32)
        n412 = local read "_HideHeader"() -> (w946:bool)
        n413 = Multiply(x=w942, y=u32 2) -> (x*y=w965:u32)
        n414 = case shown="1" w943 {
          selector: w943 -> [_ w1009 _]
          tunnel: w940 -> [_ _ _]
          tunnel: w941 -> [_ w1014 w1017]
          tunnel: [32 ("ImageRows(32)") w1008 w1018] -> w939
          tunnel: w971 -> [_ w1012 _]
          tunnel: w965 -> [_ w1011 w1015]
          frame 0 {
          }
          frame Default {
            n415 = Decrement(x=w1009) -> ()  [unwired: 1 out]
            n416 = Array Subset(array=w1014, length=w1009) -> (w1013:i32[])  [unwired: 1 in]
            n417 = Add Array Elements(numeric array=w1013) -> (sum=w1008:i32)
            n418 = Increment(x=w1011) -> (x+1=w1010:u32)
            n419 = Compound Arithmetic op=ADD(w1010, w1012, w1008) -> ()  [unwired: 1 out]
          }
          frame 1 {
            n420 = Index Array(array=w1017) -> (element=w1016:i32)  [unwired: 1 in]
            n421 = Compound Arithmetic op=ADD(w1015, w1016) -> (w1018:u32)
          }
        }
        n422 = stacked-sequence {
          tunnel: w956 -> [w1001]
          tunnel: [w1001] -> w955
          tunnel: [w1000] -> w951
          frame #0 {
            n423 = Tick Count (ms)() -> (millisecond timer value=w1000:u32)
          }
        }
        n424 = call <resource>:"GDSIconEditor_IconSizeAdjustment.vi"("BodyIconHeightIn"=w940, "HideHeader"=w946, "ConnectorPaneHeight"=w941, "Frame thickness"=w942, "_IconSize"=w943, "HeaderIconIn"=w944) -> ("HeaderIconOut"=w938:u8[][], "ImageRows"=w937:i32)  [unwired: 3 in, 1 out]
        n425 = Select(t=u8[][] [], s=w946, f=w945) -> ()  [unwired: 1 out]
        n426 = Always Copy(1:w939) -> ()  [unwired: 1 out]
        n427 = call <resource>:"GDSLvIcon_CreateIconPicture.vi"("FrameColor"=w970, "FrameThickness(1)"=w974, "HeaderIconIn"=w938, "BodyIconIn"=w962, "error in (no error)"=w955, "ImageRows(32)"=w937, "BigSizeIcon(x6)"=4, "RowStart(0)"=w947, "BgIcon"=w959, "0px Splitter(False)"=w936) -> ("WholeIconOut"=w958:u8[][], "IconPictureOut"=w964:picture, "LargeIconPictureOut(x6)"=w963:picture, "error out"=w954:errorcluster)  [unwired: 4 in, 2 out]
        n428 = local write "_IconPreview"(w963) -> ()
        n429 = local write "_After"(w964) -> ()
        n430 = case shown="Default" w957 {
          tunnel: ["ShowLayoutChange" ("item tag") w1004] -> w976
          tunnel: w949 -> [_ w1003]
          frame "UpdateIcon,ShowLayoutChange" {
          }
          frame Default {
            n431 = case shown="False" w1003 {
              tunnel: ["Idle" ("item tag") "Apply icon"] -> w1004
              frame False {
              }
              frame True {
              }
            }
          }
        }
        n432 = Bundle By Name(cluster=w961, "CurrentIcon"=w959, "IconOut"=w958, "RowStart(0)"=w947, "ImageRows(32)"=w937) -> (w960:T6)
        n433 = stacked-sequence {
          tunnel: w954 -> [w999]
          tunnel: [w999] -> w953
          tunnel: [w998] -> w952
          frame #0 {
            n434 = Tick Count (ms)() -> (millisecond timer value=w998:u32)
          }
        }
        n435 = Subtract(x=w952, y=w951) -> (x-y=w950:u32)
      }
      frame "ShowLayoutChange" {
        (unwired) u16 1 items=["Full", "1 c-term high", "2 c-term high", "3 c-term high"] ("_IconSize")
        n436 = Unbundle By Name(w1025) -> ("TermWindowOpen"=w1023:bool, "NoControlsToMove"=w1027:bool, "StartIconSize"=w1030:u16)
        n437 = Unbundle By Name(w1025) -> ("ViRef"=w1036:refnum<vi>)
        n438 = local read "_IconSize"() -> (w1034:u16)
        n439 = Equal To 0?(x=w1030) -> (x = 0?=w1031:bool)
        n440 = Equal To 0?(x=w1034) -> (x = 0?=w1035:bool)
        n441 = Select(t=u16 6, s=w1031, f=w1030) -> (s? t:f=w1028:u16)
        n442 = Select(t=u16 6, s=w1035, f=w1034) -> (s? t:f=w1029:u16)
        n443 = Less?(x=w1029, y=w1028) -> (x < y?=w1026:bool)
        n444 = Compound Arithmetic op=AND(invert w1027, w1026) -> (w1022:bool)
        n445 = case shown="True" w1022 {
          tunnel: w1039 -> [w1043 w1051]
          tunnel: [w1042 w1049] -> w1038
          tunnel: w1037 -> [w1045 w1050]
          tunnel: w1036 -> [_ w1048]
          tunnel: w1034 -> [_ w1047]
          tunnel: w1023 -> [_ w1046]
          frame False {
            n446 = Enqueue Element(queue=w1045, element=cluster{"Message":string, "Picture":picture} {"Message"="Hide", "Picture"=bytes[0]}, error in (no error)=w1043) -> (error out=w1042:errorcluster)  [unwired: 1 in, 2 out]
          }
          frame True {
            n447 = case shown="False" w1046 {
              tunnel: w1051 -> [w1063 w1064]
              tunnel: w1050 -> [w1062 _]
              tunnel: [w1058 w1064] -> w1049
              tunnel: w1048 -> [w1057 _]
              tunnel: w1047 -> [w1056 _]
              frame False {
                n448 = call <resource>:"GOOP_GetControlRearrangement.vi"("VI Refnum"=w1057, "_IconSize"=w1056, "error in (no error)"=w1063) -> ("LayoutPicture"=w1061:picture, "error out"=w1059:errorcluster)  [unwired: 10 in, 5 out]
                n449 = Select(t=cluster{"Message":string, "Picture":picture} {"Message"="ShowLeftSide", "Picture"=bytes[0]} ("element"), s=FALSE, f=cluster{"Message":string, "Picture":picture} {"Message"="ShowRightSide", "Picture"=bytes[0]} ("element")) -> (s? t:f=w1052:cluster{"Message":string, "Picture":picture})
                n450 = Bundle By Name(cluster=w1052, "Picture"=w1061) -> (w1060:cluster{"Message":string, "Picture":picture})
                n451 = Enqueue Element(queue=w1062, element=w1060, error in (no error)=w1059) -> (error out=w1058:errorcluster)  [unwired: 1 in, 2 out]
              }
              frame True {
              }
            }
          }
        }
        n452 = Bundle By Name(cluster=w1025, "LayoutChangeExist"=w1022, "TermWindowOpen"=w1022) -> (w1024:T6)
        n453 = case shown="True" w1020 {
          tunnel: ["Idle" ("item tag") "Apply icon"] -> w1021
          frame False {
          }
          frame True {
          }
        }
      }
      frame "", "Idle" {
        n454 = local read "_VIPath"() -> (w1085:path)
        n455 = Unbundle By Name(w1083) -> ("IconSelected"=w1069:i32, "IconDropped"=w1070:i32, "Icon exist"=w1084:bool)
        n456 = Not A Number/Path/Refnum?(number/path/refnum=w1085) -> (NaN/Path/Refnum?=w1095:bool)
        n457 = Empty String/Path?(string/path=w1085) -> (empty?=w1094:bool)
        n458 = local read "_ApplyHeaderToAll"() -> (w1081:bool)
        n459 = Compound Arithmetic op=AND(invert w1095, invert w1094) -> (w1074:bool)
        n460 = Not(x=w1074) -> (.not. x?=w1091:bool)
        n461 = Not(x=w1074) -> (.not. x?=w1073:bool)
        n462 = And(x=w1084, y=w1074) -> (x .and. y?=w1086:bool)
        n463 = property on="_ViNotSavedMessage" class="Str"("Visible"=w1073) -> ()  [unwired: 2 in, 2 out]
        n464 = Select(t=u8 0 ("Disabled"), s=w1091, f=u8 2) -> (s? t:f=w1088:u8)
        n465 = property class="VI"("Front Panel.Open"=TRUE ("Front Panel Window:Open")) -> ()  [unwired: 2 in, 2 out]
        n466 = Select(t=u8 2 ("Disabled"), s=w1073, f=u8 0) -> (s? t:f=w1077:u8)
        n467 = Select(t=u8 0 ("Disabled"), s=w1086, f=u8 2) -> (s? t:f=w1087:u8)
        n468 = property on="_VIPath" class="Path"("Disabled"=w1088) -> ()  [unwired: 2 in, 2 out]
        n469 = property on="_ApplyHeaderToAll" class="Bool (strict)"("Disabled"=w1077) -> ()  [unwired: 2 in, 2 out]
        n470 = Select(t=1000, s=w1081, f=-1) -> (s? t:f=w1080:i32)
        n471 = property on="Accept" class="Bool"("Disabled"=w1087) -> ()  [unwired: 2 in, 2 out]
        n472 = event shown="[7] \"_EditHeader\": Value Change" {
          selector: _ -> [_ _ _ _ _ _ _ _ _ _ _ _ _ _ _ _ _ _ _ _ _ _ _ _ _ _ _ _ _ _ _ _ _ _ _ _]
          dyn-events: _ -> [_ _ _ _ _ _ _ _ _ _ _ _ _ _ _ _ _ _ _ _ _ _ _ _ _ _ _ _ _ _ _ _ _ _ _ _]
          timeout: w1080 -> [_ _ _ _ _ _ _ _ _ _ _ _ _ _ _ _ _ _ _ _ _ _ _ _ _ _ _ _ _ _ _ _ _ _ _ _]
          tunnel: [w1103 "Generate icon" "Idle" "Generate icon" "UseBeforePicture" ("t") "Generate icon" "Exit" w1188 "ReadIcons" "Idle" w1223 _ _ w1316 w1329 "DrawIcons:NoBusy" ("y") "Generate icon" w1359 "Generate icon" _ _ "DoIconTextOCR" ("t") "Template VI" "AnalyseFileName" "Apply icon" "GetImageData" ("y") "Idle" ("t") "Idle" ("t") "UpdateIcon" ("y") w1439 _ w1479 _ w1534 "Exit" "UpdateApplyToAllText"] -> w1096
          tunnel: w1083 -> [w1099 _ _ _ w1153 _ _ w1186 _ _ w1206 w1265 w1274 w1315 _ _ _ _ _ _ _ _ _ w1395 _ _ w1419 _ w1433 w1437 _ w1477 _ w1540 _ _]
          tunnel: w1083 -> [w1102 w1113 w1119 w1144 w1155 w1165 w1181 w1187 w1198 w1201 w1225 w1267 w1277 w1312 w1331 w1349 w1353 w1356 w1362 w1365 w1368 w1372 w1375 w1390 w1397 w1415 w1417 w1426 w1430 w1441 w1474 w1483 w1523 w1539 w1582 w1586]
          tunnel: [w1101 w1114 w1119 w1143 w1155 w1165 w1181 w1187 w1198 w1201 w1224 w1266 w1276 w1311 w1330 w1349 w1352 w1356 w1362 w1365 w1368 w1372 w1375 w1385 w1397 w1414 w1417 w1425 w1429 w1440 w1474 w1482 w1522 w1538 w1582 w1586] -> w1082
          tunnel: w1072 -> [_ _ _ _ _ _ _ _ _ _ _ _ _ _ _ _ _ _ _ _ _ _ _ _ _ _ _ _ _ _ _ _ _ _ _ _]
          tunnel: w1071 -> [_ _ _ _ _ _ _ _ _ _ _ _ _ _ _ _ _ _ _ _ _ _ _ _ _ _ _ _ _ _ _ _ _ _ _ _]
          tunnel: w1070 -> [_ _ _ _ _ _ _ _ _ _ _ _ _ _ _ _ _ _ _ _ _ _ _ _ _ _ _ _ _ _ _ _ _ _ _ _]
          tunnel: w1069 -> [_ _ _ _ _ _ _ _ _ _ _ _ _ _ _ _ _ _ _ _ _ _ _ _ _ _ _ _ _ _ _ _ _ _ _ _]
          tunnel: w1067 -> [w1097 w1117 w1118 w1135 w1151 w1164 w1180 w1183 w1197 w1200 w1205 w1262 w1272 w1314 w1338 w1347 w1350 w1355 w1361 w1364 w1367 w1370 w1374 w1377 w1396 w1399 w1416 w1422 w1427 w1435 w1473 w1475 w1520 w1524 w1581 w1585]
          tunnel: [w1097 w1117 w1118 w1135 w1151 w1164 w1180 w1183 w1197 w1200 w1205 w1262 w1272 w1313 w1338 w1347 w1350 w1355 w1361 w1364 w1367 w1370 w1374 w1377 w1396 w1399 w1416 w1422 w1427 w1435 w1473 w1475 w1520 w1524 w1581 w1585] -> w1066
          tunnel: w1065 -> [_ w1108 _ _ _ _ _ _ _ _ _ _ _ w1278 _ _ _ _ _ _ _ _ _ _ _ _ _ _ _ _ _ _ _ _ _ _]
          event "_ApplyHeaderToAll": Value Change {
            n473 = event-data() -> ()  [unwired: 1 in, 6 out]
            n474 = Unbundle By Name(w1099) -> ("Text0"=w1098:string)
            n475 = case shown="True" "_ApplyHeaderToAll" {
              tunnel: ["Idle" "UpdateApplyToAllText"] -> w1103
              tunnel: w1098 -> [w1105 _]
              frame False {
                n476 = property on="_ApplyHeaderToAll" class="Bool (strict)"("BoolText.Text"=w1105) -> ()  [unwired: 2 in, 2 out]
              }
              frame True {
              }
            }
            n477 = Bundle By Name(cluster=w1102, "Counter"=0) -> (w1101:T6)
          }
          event "ClearIcon": Value Change {
            w1111 = FALSE ("Visible")
            n478 = event-data() -> ()  [unwired: 1 in, 6 out]
            n479 = property on="ClearIcon" class="Bool"("Visible"=w1111) -> ()  [unwired: 2 in, 2 out]
            n480 = Not(x=w1111) -> (.not. x?=w1110:bool)
            n481 = And(x=w1110, y=w1108) -> (x .and. y?=w1109:bool)
            n482 = property on="QuickIcons" class="Ring (strict)"("Visible"=w1109) -> ()  [unwired: 2 in, 2 out]
            n483 = Bundle By Name(cluster=w1113, "BodyIcon"=u8[][] [], "CurrentIcon"=T13 {"BgIcon"=[], "BgIconOffset"={"X"=0, "Y"=0}, "BgIconMask"=[], "ColorsOkayforiconToBeOnTopOf"=[]}) -> (w1114:T6)
          }
          event Mouse Enter; Mouse Leave {
            n484 = event-data() -> ("CtlRef"=w1128:refnum<vi>, "Type"=w1123:T14)  [unwired: 1 in]
            n485 = property class="Clust (strict)"(reference=w1128) -> (reference out=w1127:refnum<vi>, error out=w1126:errorcluster, "Value"=w1125:T24)  [unwired: 1 in]
            n486 = Equal?(x=w1123, y=lveventtype."Mouse Enter") -> (x = y?=w1121:bool)
            n487 = Bundle By Name(cluster=w1125, "Decal"=w1121) -> (w1124:T24)
            n488 = property class="Clust (strict)"(reference=w1127, error in=w1126, "Value"=w1124) -> ()  [unwired: 2 out]
          }
          event Value Change {
            n489 = event-data() -> ("OldVal"=w1140:T2)  [unwired: 1 in, 5 out]
            n490 = local read "_BodyTextColor"() -> (w1130:T2)
            n491 = Unbundle("_BackgroundColor") -> ("Color"=w1136:u32)  [unwired: 1 out]
            n492 = Unbundle(w1140) -> ("Color"=w1138:u32)  [unwired: 1 out]
            n493 = call <resource>:"GDSLvIcon_Convert24bitTo8bitColor.vi"("Color 24bit In"=w1136) -> ("Adjusted 24bit Color Out"=w1129:u32, "Color out(256)"=w1131:u8)  [unwired: 15 in, 2 out]
            n494 = Unbundle By Name(w1144) -> ("CurrentIcon.ColorsOkayforiconToBeOnTopOf"=w1145:u8[])
            n495 = call <resource>:"GDSLvIcon_Convert24bitTo8bitColor.vi"("Color 24bit In"=w1138) -> ("Color out(256)"=w1137:u8)  [unwired: 15 in, 3 out]
            n496 = Unbundle By Name(w1130) -> ("Color"=w1133:u32)
            n497 = Search 1D Array(1D array=w1145, element=w1137) -> (index of element=w1141:i32)  [unwired: 1 in]
            n498 = call <resource>:"GDSLvIcon_Convert24bitTo8bitColor.vi"("Color 24bit In"=w1133) -> ("Color out(256)"=w1132:u8)  [unwired: 15 in, 3 out]
            n499 = Replace Array Subset(array=w1145, new element=w1131, index=w1141) -> (w1142:u8[])
            n500 = Equal?(x=w1131, y=w1132) -> (x = y?=w1134:bool)
            n501 = case shown="True" w1134 {
              tunnel: w1129 -> [_ w1148]
              tunnel: w1130 -> [_ w1150]
              frame False {
              }
              frame True {
                n502 = call <resource>:"GDSLvIcon_CalculateBrightness.vi"("RGB Color In"=w1148) -> ("SuggestedTextColor"=w1147:u32)  [unwired: 8 in, 2 out]
                n503 = Bundle By Name(cluster=w1150, "Color"=w1147) -> (w1149:T2)
                n504 = local write "_BodyTextColor"(w1149) -> ()
              }
            }
            n505 = Bundle By Name(cluster=w1144, "CurrentIcon.ColorsOkayforiconToBeOnTopOf"=w1142) -> (w1143:T6)
          }
          event "_Before": Mouse Down {
            n506 = event-data() -> ()  [unwired: 1 in, 8 out]
            n507 = Unbundle By Name(w1153) -> ("StartIconSize"=w1152:u16)
            n508 = local write "_IconSize"(w1152) -> ()
          }
          event "_FontCompression", "_FontCapitalOnly": Value Change {
            n509 = event-data() -> ()  [unwired: 1 in, 2 out]
            n510 = local read "_BackgroundColor"() -> (w1156:T2)
            n511 = Unbundle By Name("_BodyTextColor") -> ("Color"=w1161:u32)
            n512 = Unbundle By Name(w1156) -> ("Color"=w1159:u32)
            n513 = call <resource>:"GDSLvIcon_Convert24bitTo8bitColor.vi"("Color 24bit In"=w1161) -> ("Adjusted 24bit Color Out"=w1157:u32, "Color out(256)"=w1160:u8)  [unwired: 15 in, 2 out]
            n514 = call <resource>:"GDSLvIcon_Convert24bitTo8bitColor.vi"("Color 24bit In"=w1159) -> ("Color out(256)"=w1158:u8)  [unwired: 15 in, 3 out]
            n515 = Equal?(x=w1160, y=w1158) -> (x = y?=w1162:bool)
            n516 = case shown="True" w1162 {
              tunnel: w1157 -> [_ w1179]
              tunnel: w1156 -> [_ w1171]
              frame False {
              }
              frame True {
                n517 = call <vilib>:"Color to RGB.vi"("Color"=w1179) -> ("R"=w1178:u8, "G"=w1177:u8, "B"=w1176:u8)  [unwired: 1 out]
                n518 = Build Array(w1178, w1177, w1176) -> (w1175:u8[])
                n519 = call-poly <vilib>:"Mean.vi"("X"=w1175) -> ("mean"=w1174:dbl)  [unwired: 1 out]
                n520 = Greater Or Equal?(x=w1174, y=128.0) -> (x >= y?=w1172:bool)
                n521 = Select(t=u32 0 ("Color"), s=w1172, f=u32 16777215 ("Color")) -> (s? t:f=w1167:u32)
                n522 = Bundle By Name(cluster=w1171, "Color"=w1167) -> (w1170:T2)
                n523 = local write "_BackgroundColor"(w1170) -> ()
              }
            }
          }
          event "_Cancel": Value Change {
            n524 = event-data() -> ()  [unwired: 1 in, 2 out]
          }
          event "_EditHeader": Value Change {
            n525 = event-data() -> ()  [unwired: 1 in, 2 out]
            n526 = Unbundle By Name(w1186) -> ("LibraryRef"=w1185:refnum<vi>)
            n527 = Not A Number/Path/Refnum?(number/path/refnum=w1185) -> (NaN/Path/Refnum?=w1184:bool)
            n528 = case shown="True" w1184 {
              tunnel: [w1193 "Edit header"] -> w1188
              frame False {
                w1190 = "Edit VI Header"  # _Edit VI Header
                w1191 = "Edit Library Header"  # _Edit Library Header
                w1192 = "This VI belongs to a library and you can decide if you want to modify the library file's header or just this VI's header."  # _LibraryEditHeaderQuestion
                n529 = Two Button Dialog(message=w1192, 1:w1190, 2:w1191) -> (T button?=w1189:bool)
                n530 = case shown="False" w1189 {
                  tunnel: ["Edit header" "Edit Library Header"] -> w1193
                  frame False {
                  }
                  frame True {
                  }
                }
              }
              frame True {
              }
            }
          }
          event "_Folders": Value Change {
            n531 = event-data() -> ()  [unwired: 1 in, 1 out]
          }
          event "_HelpCreateClass": Value Change {
            n532 = event-data() -> ()  [unwired: 1 in, 6 out]
            n533 = fn#1354() -> (1:w1204:bool)  [unwired: 1 out]
            n534 = Not(x=w1204) -> (.not. x?=w1203:bool)
            n535 = Control Help Window(1:w1203) -> ()  [unwired: 1 in]
          }
          event "_IconPreview": Mouse Down {
            w1209 = 4 ("y")
            # "Check if Mouse down on text, if so Start dragging Text"
            n536 = event-data() -> ("Coords"=w1222:T5)  [unwired: 1 in]
            n537 = property on="_IconPreview" class="Pict"() -> ("Mouse"=w1213:T25)  [unwired: 2 in, 2 out]
            n538 = Unbundle By Name(w1213) -> ("Mouse Position.X"=w1210:i32, "Mouse Position.Y"=w1212:i32)
            n539 = Unbundle By Name(w1206) -> ("IconDropped"=w1221:i32, "TextBounds"=w1220:T23)
            n540 = Unbundle(w1220) -> ("FirstRow"=w1218:i32, "FirstColumn"=w1217:i32, "LastRow"=w1219:i32, "LastColumn"=w1214:i32)
            n541 = Divide(x=w1210, y=w1209) -> (x/y=w1208:dbl)
            n542 = Divide(x=w1212, y=w1209) -> (x/y=w1211:dbl)
            n543 = In Range and Coerce(upper limit=w1219, x=w1211, lower limit=w1218) -> (In Range?=w1216:bool)  [unwired: 1 out]
            n544 = In Range and Coerce(upper limit=w1214, x=w1208, lower limit=w1217) -> (In Range?=w1215:bool)  [unwired: 1 out]
            n545 = And(x=w1216, y=w1215) -> (x .and. y?=w1207:bool)
            n546 = case shown="True" w1207 {
              tunnel: w1225 -> [w1230 w1261]
              tunnel: [w1229 w1258] -> w1224
              tunnel: [w1228 "Idle" ("y")] -> w1223
              tunnel: w1222 -> [w1227 w1252]
              tunnel: w1221 -> [w1226 _]
              tunnel: w1206 -> [_ w1256]
              frame False {
                n547 = case shown="Default" w1226 {
                  selector: w1226 -> [_ w1233]
                  tunnel: w1230 -> [w1232 w1248]
                  tunnel: [w1232 w1247] -> w1229
                  tunnel: ["Idle" ("y") "ShowDragIcon:UpdateIcon" ("y")] -> w1228
                  tunnel: w1227 -> [_ w1234]
                  frame Default {
                  }
                  frame 0.. {
                    n548 = property on="DragIcon" class="Pict"() -> ("Draw Area Size"=w1245:T7)  [unwired: 2 in, 2 out]
                    n549 = Divide(x=w1245, y=2) -> (x/y=w1243:cluster{"Width":dbl, "Height":dbl})
                    n550 = Subtract(x=w1234, y=w1243) -> (x-y=w1237:cluster{dbl, dbl})
                    n551 = property on="_IconPreview" class="Pict"() -> ("Position"=w1241:T15)  [unwired: 2 in, 2 out]
                    n552 = property on="DragIcon" class="Pict"("Position"=w1237) -> ()  [unwired: 2 in, 2 out]
                    n553 = Add(x=w1241, y=T15 {"Left"=0, "Top"=16}) -> (x+y=w1240:T15)
                    n554 = Subtract(x=w1237, y=w1240) -> (x-y=w1238:cluster{dbl, dbl})
                    n555 = Divide(x=w1238, y=u8 4 ("Disabled")) -> (x/y=w1236:cluster{dbl, dbl})
                    n556 = Bundle By Name(cluster=w1248, "IconSelected"=w1233, "DraggingIcon"=TRUE ("Draging"), "BgIconOffset"=w1236) -> (w1247:T6)
                  }
                }
              }
              frame True {
                n557 = Unbundle By Name(w1256) -> ("Offset.X"=w1255:i32, "Offset.Y"=w1254:i32)
                n558 = Bundle("X"=w1255, "Y"=w1254) -> (w1250:cluster{"X":i32, "Y":i32})  [unwired: 1 in]
                n559 = Multiply(x=w1250, y=4) -> (x*y=w1249:cluster{"X":i32, "Y":i32})
                n560 = Subtract(x=w1252, y=w1249) -> (x-y=w1251:T5)
                n561 = Bundle By Name(cluster=w1261, "DraggingIcon"=FALSE, "DraggingText"=TRUE, "StartTextDraggingPos"=w1251) -> (w1258:T6)
              }
            }
          }
          event "_IconPreview": Mouse Enter {
            n562 = event-data() -> ()  [unwired: 1 in, 1 out]
            n563 = Unbundle By Name(w1265) -> ("DraggingIcon"=w1263:bool, "IconDropped"=w1264:i32)
            n564 = case shown="True" w1263 {
              tunnel: w1267 -> [w1270 w1271]
              tunnel: [w1269 w1271] -> w1266
              tunnel: w1264 -> [w1268 _]
              frame False {
                n565 = Bundle By Name(cluster=w1270, "IconSelected"=w1268) -> (w1269:T6)
              }
              frame True {
              }
            }
          }
          event "_IconPreview": Mouse Up {
            w1275 = FALSE ("Draging")
            n566 = event-data() -> ()  [unwired: 1 in, 3 out]
            n567 = Unbundle By Name(w1274) -> ("IconSelected"=w1273:i32)
            n568 = Bundle By Name(cluster=w1277, "IconDropped"=w1273, "Moving"=w1275, "DraggingIcon"=w1275) -> (w1276:T6)
            n569 = property on="DragIcon" class="Pict"("Visible"=w1275) -> ()  [unwired: 2 in, 2 out]
          }
          event "_Icons": Value Change {
            n570 = event-data() -> ()  [unwired: 1 in, 1 out]
            n571 = Unbundle By Name(w1315) -> ("HeaderIcon"=w1303:u8[][])
            n572 = Unbundle By Name(w1315) -> ("RowStart(0)"=w1299:i32, "ImageRows(32)"=w1298:i32, "Frame thickness"=w1300:i32, "FrameColor"=w1297:u32)
            n573 = Unbundle By Name(w1315) -> ("BodyIconHeight"=w1288:i32, "BodyIconWidth"=w1287:i32, "HeaderBkColor"=w1286:u32, "Offset"=w1280:cluster{"X":i32, "Y":i32}, "CurrentIcon"=w1279:T13)
            n574 = local read "_IconSize"() -> (w1308:u16)
            n575 = local read "_HideHeader"() -> (w1305:bool)
            n576 = local read "_BackgroundColor"() -> (w1292:T2)
            n577 = local read "_BodyTextColor"() -> (w1291:T2)
            n578 = Equal?(x=w1308, y=u16 1) -> (x = y?=w1306:bool)
            n579 = local read "_MethodIconName"() -> (w1296:string)
            n580 = local read "_FontCapitalOnly"() -> (w1295:bool)
            n581 = local read "_FontCompression"() -> (w1294:enum16{"Auto", "On", "Off"})
            n582 = local read "_TextAlignment"() -> (w1293:u16)
            n583 = Or(x=w1305, y=w1306) -> (x .or. y?=w1304:bool)
            n584 = Unbundle By Name(w1291) -> ("Color"=w1290:u32)
            n585 = Unbundle By Name(w1292) -> ("Color"=w1289:u32)
            n586 = Select(t=u8[][] [], s=w1304, f=w1303) -> (s? t:f=w1301:u8[][])
            n587 = Bundle By Name(cluster=T16 {"HeaderIcon"=[], "RowStart(0)"=0, "ImageRows(32)"=32, "FrameThickness(1)"=1, "FrameColor"=0, "IconTextDataType"={"Text"="", "Allow Only Capital Chars"=FALSE, "Compression"=enum."Auto", "Alignment"=enum."Center"}, "BodyTextColor"=0, "BodyBackgroundColor"=0, "BodyIconHeight"=0, "BodyIconWidth"=0, "HeaderBackgroundColor"=0, "BodyIcon"=[[0, 0, 0, 0, 0, 0, 0, 0, 0, 0, 255, 255, 0, 0, 255, 0, 0, 0, 255, 0, 0, 0, 0, 0, 0, 0, 0, 0, 0, 0], [0, 0, 0, 0, 0, 0, 0, 0, 0, 255, 0, 0, 255, 0, 255, 0, 0, 0, 255, 0, 0, 0, 0, 0, 0, 0, 0, 0, 0, 0], [0, 0, 0, 0, 0, 0, 0, 0, 0, 255, 255, 255, 255, 0, 255, 0, 0, 0, 255, 0, 0, 0, 0, 0, 0, 0, 0, 0, 0, 0], [0, 0, 0, 0, 0, 0, 0, 0, 0, 255, 0, 0, 255, 0, 255, 0, 0, 0, 255, 0, 0, 0, 0, 0, 0, 0, 0, 0, 0, 0], [0, 0, 0, 0, 0, 0, 0, 0, 0, 255, 0, 0, 255, 0, 255, 255, 255, 0, 255, 255, 255, 0, 0, 0, 0, 0, 0, 0, 0, 0], [0, 0, 255, 0, 0, 0, 255, 0, 0, 255, 255, 0, 0, 255, 0, 0, 255, 0, 255, 255, 0, 255, 255, 0, 0, 0, 255, 255, 0, 0], [0, 255, 0, 255, 0, 255, 0, 255, 0, 255, 0, 255, 0, 255, 255, 0, 255, 0, 255, 0, 0, 255, 0, 255, 0, 255, 0, 0, 0, 0], [0, 255, 0, 0, 0, 255, 0, 255, 0, 255, 255, 0, 0, 255, 0, 255, 255, 0, 255, 255, 0, 255, 255, 0, 0, 0, 255, 0, 0, 0], [0, 255, 0, 255, 0, 255, 0, 255, 0, 255, 0, 255, 0, 255, 0, 0, 255, 0, 255, 0, 0, 255, 0, 255, 0, 0, 0, 255, 0, 0], [0, 0, 255, 0, 0, 0, 255, 0, 0, 255, 0, 255, 0, 255, 0, 0, 255, 0, 255, 255, 0, 255, 0, 255, 0, 255, 255, 0, 0, 0], [0, 255, 0, 0, 0, 255, 0, 0, 255, 0, 0, 255, 0, 255, 0, 0, 255, 0, 255, 255, 0, 0, 255, 0, 0, 255, 255, 255, 0, 255], [255, 0, 255, 0, 255, 0, 255, 0, 255, 255, 0, 255, 0, 255, 255, 0, 255, 0, 255, 0, 0, 255, 0, 255, 0, 0, 255, 0, 0, 255], [255, 0, 0, 0, 255, 0, 255, 0, 255, 0, 255, 255, 0, 255, 0, 255, 255, 0, 255, 255, 0, 255, 0, 0, 0, 0, 255, 0, 0, 255], [255, 0, 255, 0, 255, 0, 255, 0, 255, 0, 0, 255, 0, 255, 0, 0, 255, 0, 255, 0, 0, 255, 0, 255, 0, 0, 255, 0, 0, 255], [0, 255, 0, 0, 0, 255, 0, 0, 255, 0, 0, 255, 0, 255, 0, 0, 255, 0, 255, 255, 0, 0, 255, 0, 0, 0, 255, 0, 0, 255], [0, 0, 0, 0, 0, 0, 0, 0, 0, 0, 0, 0, 0, 0, 255, 0, 0, 0, 0, 0, 0, 0, 0, 0, 0, 0, 0, 0, 0, 0], [0, 0, 0, 0, 0, 0, 0, 0, 0, 0, 0, 0, 0, 255, 0, 0, 0, 0, 0, 0, 0, 0, 0, 0, 0, 0, 0, 0, 0, 0], [0, 0, 0, 0, 0, 0, 0, 0, 0, 0, 0, 0, 0, 255, 255, 0, 0, 0, 0, 0, 0, 0, 0, 0, 0, 0, 0, 0, 0, 0], [0, 0, 0, 0, 0, 0, 0, 0, 0, 0, 0, 0, 0, 255, 0, 255, 0, 0, 0, 0, 0, 0, 0, 0, 0, 0, 0, 0, 0, 0], [0, 0, 0, 0, 0, 0, 0, 0, 0, 0, 0, 0, 0, 0, 255, 0, 0, 0, 0, 0, 0, 0, 0, 0, 0, 0, 0, 0, 0, 0], [0, 0, 0, 0, 0, 0, 0, 0, 0, 0, 0, 0, 0, 0, 0, 0, 0, 0, 0, 0, 0, 0, 0, 0, 0, 0, 0, 0, 0, 0], [0, 0, 0, 0, 0, 0, 0, 0, 0, 0, 0, 0, 0, 0, 0, 0, 0, 0, 0, 0, 0, 0, 0, 0, 0, 0, 0, 0, 0, 0]], "Offset"={"X"=0, "Y"=0}, "CurrentIcon"={"BgIcon"=[], "BgIconOffset"={"X"=0, "Y"=0}, "BgIconMask"=[], "ColorsOkayforiconToBeOnTopOf"=[]}} ("IconInfo"), "HeaderIcon"=w1301, "RowStart(0)"=w1299, "ImageRows(32)"=w1298, "FrameThickness(1)"=w1300, "FrameColor"=w1297, "IconTextDataType.Text"=w1296, "IconTextDataType.Allow Only Capital Chars"=w1295, "IconTextDataType.Compression"=w1294, "IconTextDataType.Alignment"=w1293, "BodyTextColor"=w1290, "BodyBackgroundColor"=w1289, "BodyIconHeight"=w1288, "BodyIconWidth"=w1287, "HeaderBackgroundColor"=w1286, "Offset"=w1280, "CurrentIcon"=w1279) -> (w1309:T16)
            n588 = call <resource>:"GDSIconEditor_IconDialog.vi"("error in (no error)"=w1314, "IconInfo"=w1309) -> ("error out"=w1313:errorcluster, "Icon exist"=w1281:bool, "CurrentIcon"=w1282:T13, "Cancelled"=w1283:bool, "Offset"=w1284:cluster{"X":i32, "Y":i32}, "BodyIcon"=w1285:u8[][])  [unwired: 4 in]
            n589 = case shown="False" w1283 {
              tunnel: w1312 -> [w1326 w1327]
              tunnel: [w1325 w1327] -> w1311
              tunnel: w1285 -> [w1324 _]
              tunnel: w1284 -> [w1323 _]
              tunnel: w1282 -> [w1322 _]
              tunnel: w1281 -> [w1320 _]
              tunnel: ["Generate icon" _] -> w1316
              tunnel: w1278 -> [w1317 _]
              frame False {
                n590 = property on="ClearIcon" class="Bool"("Visible"=w1320) -> ()  [unwired: 2 in, 2 out]
                n591 = Bundle By Name(cluster=w1326, "BodyIcon"=w1324, "Offset"=w1323, "CurrentIcon"=w1322, "Icon exist"=w1320) -> (w1325:T6)
                n592 = Not(x=w1320) -> (.not. x?=w1319:bool)
                n593 = And(x=w1319, y=w1317) -> (x .and. y?=w1318:bool)
                n594 = property on="QuickIcons" class="Ring (strict)"("Visible"=w1318) -> ()  [unwired: 2 in, 2 out]
              }
              frame True {
              }
            }
          }
          event "QuickIcons": Value Change {
            n595 = event-data() -> ()  [unwired: 1 in, 6 out]
            n596 = property on="QuickIcons" class="Ring (strict)"() -> ("Strings []"=w1335:string[])  [unwired: 2 in, 2 out]
            n597 = Array Size(array=w1335) -> (size(s)=w1334:i32)
            n598 = expression code="x-3"(w1334) -> (w1333:i32)
            n599 = In Range and Coerce(upper limit=w1333, x="QuickIcons", lower limit=u16 1) -> (In Range?=w1332:bool)  [unwired: 1 out]
            n600 = case shown="True" w1332 {
              tunnel: w1331 -> [w1340 w1346]
              tunnel: [w1340 w1345] -> w1330
              tunnel: ["" "Generate icon"] -> w1329
              frame False {
              }
              frame True {
                w1342 = TRUE ("Visible")
                n601 = property on="ClearIcon" class="Bool"("Visible"=w1342) -> ()  [unwired: 2 in, 2 out]
                n602 = Not(x=w1342) -> (.not. x?=w1343:bool)
                n603 = property on="QuickIcons" class="Ring (strict)"("Visible"=w1343) -> ()  [unwired: 2 in, 2 out]
                n604 = Bundle By Name(cluster=w1346, "CurrentIcon"=T13 {"BgIcon"=[[255, 255, 255, 255, 255, 255, 255, 255, 255, 255, 255, 255, 255, 255, 0], [255, 1, 1, 1, 1, 1, 1, 1, 1, 1, 1, 1, 1, 255, 249], [255, 1, 1, 1, 1, 1, 1, 1, 255, 255, 1, 1, 1, 255, 249], [255, 1, 1, 1, 1, 1, 1, 255, 255, 255, 255, 1, 1, 255, 249], [255, 1, 1, 255, 255, 255, 255, 255, 255, 1, 1, 1, 1, 255, 249], [255, 1, 1, 255, 255, 255, 255, 255, 255, 1, 1, 1, 1, 255, 249], [255, 1, 1, 1, 1, 1, 1, 255, 255, 255, 255, 1, 1, 255, 249], [255, 1, 1, 1, 1, 1, 1, 1, 255, 255, 1, 1, 1, 255, 249], [255, 1, 1, 1, 1, 1, 1, 1, 1, 1, 1, 1, 1, 255, 249], [255, 255, 255, 255, 255, 255, 255, 255, 255, 255, 255, 255, 255, 255, 249], [0, 249, 249, 249, 249, 249, 249, 249, 249, 249, 249, 249, 249, 249, 249]], "BgIconOffset"={"X"=9, "Y"=10}, "BgIconMask"=[255, 252, 255, 254, 255, 254, 255, 254, 255, 254, 255, 254, 255, 254, 255, 254, 255, 254, 255, 254, 127, 254], "ColorsOkayforiconToBeOnTopOf"=[185, 0]}, "Icon exist"=w1342) -> (w1345:T6)
              }
            }
            n605 = local write "QuickIcons"(0) -> ()
          }
          event "_IconSearchText": Value Change {
            n606 = event-data() -> ()  [unwired: 1 in, 1 out]
          }
          event "_IconSize", "_TextAlignment", "_HideHeader": Value Change {
            n607 = event-data() -> ()  [unwired: 1 in, 6 out]
            n608 = Bundle By Name(cluster=w1353, "Offset"=cluster{"X":i32, "Y":i32} {"X"=0, "Y"=0}) -> (w1352:T6)
          }
          event "_Manage": Value Change {
            n609 = event-data() -> ()  [unwired: 1 in, 1 out]
            n610 = call <resource>:"GDSLvIcon_ManageIconFolderDialog.vi"() -> ("Cancelled"=w1360:bool)  [unwired: 10 in, 1 out]
            n611 = Select(t="Idle", s=w1360, f="UpdateIconFolderList" ("y")) -> (s? t:f=w1359:string)
          }
          event "_MethodIconName": Value Change {
            n612 = event-data() -> ()  [unwired: 1 in, 6 out]
          }
          event "_OCR": Mouse Enter {
            w1366 = TRUE ("Boolean Text.Font:Bold")
            n613 = event-data() -> ()  [unwired: 1 in, 4 out]
            n614 = property on="_OCR" class="Bool (strict)"("BoolText.FontBold"=w1366, "BoolText.FontUnder"=w1366) -> ()  [unwired: 2 in, 2 out]
          }
          event "_OCR": Mouse Leave {
            w1369 = FALSE ("Boolean Text.Font:Bold")
            n615 = event-data() -> ()  [unwired: 1 in, 4 out]
            n616 = property on="_OCR" class="Bool (strict)"("BoolText.FontBold"=w1369, "BoolText.FontUnder"=w1369) -> ()  [unwired: 2 in, 2 out]
          }
          event "_OCR": Value Change {
            w1373 = FALSE ("Boolean Text.Font:Bold")
            n617 = event-data() -> ()  [unwired: 1 in, 6 out]
            n618 = property on="_OCR" class="Bool (strict)"("BoolText.FontBold"=w1373, "BoolText.FontUnder"=w1373) -> ()  [unwired: 2 in, 2 out]
          }
          event "_TemplateVI": Value Change {
            n619 = event-data() -> ()  [unwired: 1 in, 2 out]
          }
          event "_VIPath": Value Change {
            n620 = event-data() -> ()  [unwired: 1 in, 2 out]
            n621 = Unbundle By Name(w1395) -> ("ViRef"=w1394:refnum<vi>)
            n622 = invoke class="VI" method="Save.Instrument"(reference=w1394, "Path to saved file"="_VIPath") -> (reference out=w1391:refnum<vi>, error out=w1379:errorcluster)  [unwired: 4 in, 4 out]
            n623 = call <resource>:"CommonVIs_Wait.vi"("error in"=w1379) -> ("error out"=w1378:errorcluster)  [unwired: 9 in]
            n624 = property class="VI"(reference=w1391, error in=w1378) -> (error out=w1382:errorcluster, "Path"=w1387:path)  [unwired: 1 out]
            n625 = Strip Path(path=w1387) -> (stripped path=w1386:path, name=w1384:string)
            n626 = local write "_VIPath"(w1387) -> ()
            n627 = Unbundle By Name(w1382) -> ("status"=w1389:bool)
            n628 = Select(t=u8 2 ("Disabled"), s=w1382, f=u8 0) -> (s? t:f=w1383:u8)
            n629 = property on="_ApplyHeaderToAll" class="Bool (strict)"("Disabled"=w1383) -> ()  [unwired: 2 in, 2 out]
            n630 = Not(x=w1389) -> (.not. x?=w1388:bool)
            n631 = Bundle By Name(cluster=w1390, "Folder"=w1386, "VI Path"=w1387, "VI name"=w1384, "Icon exist"=w1388) -> (w1385:T6)
          }
          event "Accept": Value Change {
            n632 = event-data() -> ()  [unwired: 1 in, 2 out]
          }
          event "DragIcon": Mouse Down {
            n633 = event-data() -> ("Coords"=w1401:T5)  [unwired: 1 in]
            n634 = property on="DragIcon" class="Pict"() -> ("Draw Area Size"=w1412:T7)  [unwired: 2 in, 2 out]
            n635 = Divide(x=w1412, y=2) -> (x/y=w1410:cluster{"Width":dbl, "Height":dbl})
            n636 = property on="_IconPreview" class="Pict"() -> ("Position"=w1408:T15)  [unwired: 2 in, 2 out]
            n637 = Subtract(x=w1401, y=w1410) -> (x-y=w1404:cluster{dbl, dbl})
            n638 = Add(x=w1408, y=T15 {"Left"=0, "Top"=16}) -> (x+y=w1407:T15)
            n639 = Subtract(x=w1404, y=w1407) -> (x-y=w1405:cluster{dbl, dbl})
            n640 = Divide(x=w1405, y=u8 4 ("Disabled")) -> (x/y=w1403:cluster{dbl, dbl})
            n641 = property on="DragIcon" class="Pict"("Position"=w1404, "Visible"=TRUE) -> ()  [unwired: 2 in, 2 out]
            n642 = Bundle By Name(cluster=w1415, "DraggingIcon"=TRUE ("Draging"), "BgIconOffset"=w1403) -> (w1414:T6)
          }
          event "DragIcon": Mouse Leave {
            n643 = event-data() -> ()  [unwired: 1 in, 1 out]
            n644 = Unbundle By Name(w1419) -> ("DraggingIcon"=w1418:bool)
            n645 = case shown="False" w1418 {
              selector: w1418 -> [w1421 _]
              frame False {
                n646 = property on="DragIcon" class="Pict"("Visible"=w1421) -> ()  [unwired: 2 in, 2 out]
              }
              frame True {
              }
            }
          }
          event "DragIcon": Mouse Up {
            w1423 = FALSE ("Draging")
            n647 = event-data() -> ()  [unwired: 1 in, 3 out]
            n648 = Bundle By Name(cluster=w1426, "DraggingIcon"=w1423) -> (w1425:T6)
            n649 = property on="DragIcon" class="Pict"("Visible"=w1423) -> ()  [unwired: 2 in, 2 out]
          }
          event "FloodFillMask": Value Change {
            n650 = event-data() -> ()  [unwired: 1 in, 1 out]
            n651 = Unbundle By Name(w1433) -> ("BgIcon"=w1432:u8[][])
            n652 = call <resource>:"GDSIconEditor_CreateImageMask.vi"("Flood Fill"="FloodFillMask", "8-bit pixmap"=w1432) -> ("Array"=w1428:u8[])
            n653 = Bundle By Name(cluster=w1430, "BgIconMask"=w1428) -> (w1429:T6)
          }
          event "Icons", "DragIcon": Mouse Move {
            n654 = event-data() -> ("Coords"=w1438:T5)  [unwired: 1 in]
            n655 = Unbundle By Name(w1437) -> ("DraggingIcon"=w1436:bool)
            n656 = case shown="False" w1436 {
              tunnel: w1441 -> [w1454 w1472]
              tunnel: [w1453 w1472] -> w1440
              tunnel: [w1451 "Idle" ("t")] -> w1439
              tunnel: w1438 -> [w1449 _]
              tunnel: w1437 -> [w1446 _]
              frame False {
                n657 = Unbundle By Name(w1446) -> ("IconPos"=w1455:T26)
                n658 = property on="Icons" class="Pict"() -> ("Position"=w1450:T15)  [unwired: 2 in, 2 out]
                n659 = property on="Icons" class="Pict"() -> ("Origin"=w1445:T17)  [unwired: 2 in, 2 out]
                n660 = Subtract(x=w1449, y=w1450) -> (x-y=w1444:T5)
                n661 = Add(x=w1445, y=w1444) -> (x+y=w1443:T5)
                n662 = for {
                  tunnel: w1455 -> [w1465] mode=indexing
                  tunnel: w1443 -> [w1467]
                  tunnel: [w1457] -> w1452
                  tunnel: [w1456] -> w1448
                  i -> [w1456]
                  stop <- w1457 stop-if-true
                  n663 = Unbundle(w1465) -> ("left"=w1464:i16, "top"=w1460:i16, "right"=w1463:i16, "bottom"=w1462:i16)
                  n664 = Unbundle(w1467) -> ("Horizontal"=w1466:i32, "Vertical"=w1461:i32)
                  n665 = In Range and Coerce(upper limit=w1463, x=w1466, lower limit=w1464) -> (In Range?=w1458:bool)  [unwired: 1 out]
                  n666 = In Range and Coerce(upper limit=w1462, x=w1461, lower limit=w1460) -> (In Range?=w1459:bool)  [unwired: 1 out]
                  n667 = And(x=w1458, y=w1459) -> (x .and. y?=w1457:bool)
                }
                n668 = Select(t=w1448, s=w1452, f=-1) -> (s? t:f=w1442:i32)
                n669 = case shown="True" w1452 {
                  tunnel: ["Idle" ("t") "ShowDragIcon" ("t")] -> w1451
                  frame False {
                    n670 = property on="DragIcon" class="Pict"("Visible"=FALSE) -> ()  [unwired: 2 in, 2 out]
                  }
                  frame True {
                  }
                }
                n671 = Bundle By Name(cluster=w1454, "IconSelected"=w1442) -> (w1453:T6)
              }
              frame True {
              }
            }
          }
          event "Icons": Mouse Enter {
            n672 = event-data() -> ()  [unwired: 1 in, 1 out]
          }
          event Mouse Move {
            n673 = event-data() -> ("Coords"=w1481:T5)  [unwired: 1 in]
            n674 = Unbundle By Name(w1477) -> ("StartTextDraggingPos"=w1476:T5)
            n675 = Unbundle By Name(w1477) -> ("DraggingText"=w1478:bool, "DraggingIcon"=w1480:bool)
            n676 = case shown="True" w1480 {
              tunnel: w1483 -> [w1489 w1512]
              tunnel: [w1488 w1511] -> w1482
              tunnel: w1481 -> [w1485 w1507]
              tunnel: w1477 -> [w1484 _]
              tunnel: [w1487 "UpdateIcon" ("y")] -> w1479
              tunnel: w1478 -> [w1490 _]
              tunnel: w1476 -> [w1486 _]
              frame False {
                n677 = case shown="True" w1490 {
                  tunnel: w1489 -> [w1491 w1505]
                  tunnel: [w1491 w1504] -> w1488
                  tunnel: [_ "Generate icon"] -> w1487
                  tunnel: w1486 -> [_ w1501]
                  tunnel: w1485 -> [_ w1502]
                  tunnel: w1484 -> [_ w1500]
                  frame False {
                  }
                  frame True {
                    n678 = Subtract(x=w1502, y=w1501) -> (x-y=w1497:T5)
                    n679 = Unbundle By Name(w1500) -> ("Offset.X"=w1495:i32, "Offset.Y"=w1494:i32)
                    n680 = Divide(x=w1497, y=u8 4 ("f")) -> (x/y=w1496:cluster{"Horizontal":dbl, "Vertical":dbl})
                    n681 = Unbundle By Name(w1496) -> ("Horizontal"=w1493:dbl, "Vertical"=w1492:dbl)
                    n682 = Bundle By Name(cluster=w1505, "OldOffset.X"=w1495, "OldOffset.Y"=w1494) -> (w1499:T6)
                    n683 = Bundle By Name(cluster=w1499, "Offset.X"=w1493, "Offset.Y"=w1492) -> (w1504:T6)
                  }
                }
              }
              frame True {
                n684 = property on="DragIcon" class="Pict"() -> ("Draw Area Size"=w1517:T7)  [unwired: 2 in, 2 out]
                n685 = property on="_IconPreview" class="Pict"() -> ("Position"=w1515:T15)  [unwired: 2 in, 2 out]
                n686 = Divide(x=w1517, y=2.0 ("Waveform Chart")) -> (x/y=w1518:cluster{"Width":dbl, "Height":dbl})
                n687 = Add(x=w1515, y=T15 {"Left"=0, "Top"=16}) -> (x+y=w1514:T15)
                n688 = Subtract(x=w1507, y=w1518) -> (x-y=w1506:cluster{dbl, dbl})
                n689 = Subtract(x=w1506, y=w1514) -> (x-y=w1509:cluster{dbl, dbl})
                n690 = property on="DragIcon" class="Pict"("Position"=w1506) -> ()  [unwired: 2 in, 2 out]
                n691 = Divide(x=w1509, y=u8 4 ("Disabled")) -> (x/y=w1508:cluster{dbl, dbl})
                n692 = Bundle By Name(cluster=w1512, "BgIconOffset"=w1508) -> (w1511:T6)
              }
            }
          }
          event Mouse Up; Mouse Leave {
            w1521 = FALSE ("DraggingText")
            n693 = event-data() -> ()  [unwired: 1 in, 1 out]
            n694 = Bundle By Name(cluster=w1523, "DraggingText"=w1521) -> (w1522:T6)
            n695 = property on="DragIcon" class="Pict"("Visible"=w1521) -> ()  [unwired: 2 in, 2 out]
          }
          event Key Down? {
            (unwired) TRUE
            n696 = event-data() -> ("VKey"=w1537:T27, "PlatMods"=w1533:T28)  [unwired: 1 in, 2 out]
            n697 = property on="_FontCompression" class="Enum (strict)"() -> ("Key Focus"=w1531:bool)  [unwired: 2 in, 2 out]
            n698 = property on="_MethodIconName" class="Str"() -> ("Key Focus"=w1528:bool)  [unwired: 2 in, 2 out]
            n699 = property on="_TextAlignment" class="Ring (strict)"() -> ("Key Focus"=w1529:bool)  [unwired: 2 in, 2 out]
            n700 = property on="_IconSize" class="Ring (strict)"() -> ("Key Focus"=w1530:bool)  [unwired: 2 in, 2 out]
            n701 = Unbundle By Name(w1540) -> ("Offset.X"=w1535:i32, "Offset.Y"=w1536:i32)
            n702 = Unbundle By Name(w1533) -> ("Ctrl"=w1526:bool)
            n703 = Compound Arithmetic op=AND(invert w1531, invert w1530, invert w1529, invert w1528) -> (w1527:bool)
            n704 = Or(x=w1526, y=w1527) -> (x .or. y?=w1525:bool)
            n705 = case shown="True" w1525 {
              tunnel: w1539 -> [w1542 w1546]
              tunnel: [w1542 w1550] -> w1538
              tunnel: w1537 -> [_ w1549]
              tunnel: w1536 -> [_ w1543]
              tunnel: w1535 -> [_ w1544]
              tunnel: ["Idle" w1548] -> w1534
              tunnel: [_ w1547] -> w1532
              frame False {
              }
              frame True {
                n706 = Bundle By Name(cluster=w1546, "OldOffset.X"=w1544, "OldOffset.Y"=w1543) -> (w1545:T6)
                n707 = case shown="\"Right\"" w1549 {
                  tunnel: w1545 -> [w1557 w1559 w1566 w1573 w1580]
                  tunnel: [w1556 w1559 w1565 w1572 w1579] -> w1550
                  tunnel: w1543 -> [w1555 _ w1564 w1570 w1577]
                  tunnel: w1544 -> [w1553 _ w1562 w1571 w1578]
                  tunnel: ["Generate icon" "Idle" "Generate icon" "Generate icon" "Generate icon"] -> w1548
                  tunnel: [TRUE _ TRUE TRUE TRUE] -> w1547
                  frame "Up" {
                    n708 = Decrement(x=w1555) -> (x-1=w1554:i32)
                    n709 = Bundle By Name(cluster=w1557, "Offset.X"=w1553, "Offset.Y"=w1554) -> (w1556:T6)
                  }
                  frame Default {
                  }
                  frame "Down" {
                    n710 = Increment(x=w1564) -> (x+1=w1563:i32)
                    n711 = Bundle By Name(cluster=w1566, "Offset.X"=w1562, "Offset.Y"=w1563) -> (w1565:T6)
                  }
                  frame "Left" {
                    n712 = Decrement(x=w1571) -> (x-1=w1569:i32)
                    n713 = Bundle By Name(cluster=w1573, "Offset.X"=w1569, "Offset.Y"=w1570) -> (w1572:T6)
                  }
                  frame "Right" {
                    n714 = Increment(x=w1578) -> (x+1=w1576:i32)
                    n715 = Bundle By Name(cluster=w1580, "Offset.X"=w1576, "Offset.Y"=w1577) -> (w1579:T6)
                  }
                }
              }
            }
            n716 = event-data("Discard?"=w1532) -> ()  [unwired: 1 in, 1 out]
          }
          event Panel Close? {
            n717 = event-data() -> ()  [unwired: 1 in, 2 out]
            n718 = event-data("Discard?"=TRUE) -> ()  [unwired: 1 in, 1 out]
          }
          event Timeout {
            n719 = event-data() -> ()  [unwired: 1 in, 3 out]
          }
        }
      }
      frame "GetImageData" {
        # "Create White mask Color, When Mouse Down"
        n720 = Unbundle By Name(w1597) -> ("Icons"=w1599:T4[], "IconSelected"=w1598:i32)
        n721 = Index Array(array=w1599, index=w1598) -> (element=w1588:T4)
        n722 = call <resource>:"GDSIconEditor_ShrinkImage.vi"("image data"=w1588) -> ("image subset"=w1589:T4)  [unwired: 9 in]
        n723 = call <resource>:"GDSIconEditor_ImageDataTo8Bit.vi"("image data"=w1589) -> ("NoMaskFound"=w1590:bool, "8-bit pixmap"=w1591:u8[][], "mask"=w1595:u8[])  [unwired: 7 in, 1 out]
        n724 = property on="FloodFillMask" class="Bool (strict)"("Visible"=w1590) -> ()  [unwired: 2 in, 2 out]
        n725 = case shown="True" w1590 {
          tunnel: w1591 -> [_ w1604]
          tunnel: w1595 -> [w1601 _]
          tunnel: [w1601 w1603] -> w1592
          frame False {
          }
          frame True {
            n726 = local read "FloodFillMask"() -> (w1602:bool)
            n727 = call <resource>:"GDSIconEditor_CreateImageMask.vi"("Flood Fill"=w1602, "8-bit pixmap"=w1604) -> ("Array"=w1603:u8[])
          }
        }
        n728 = call <vilib>:"Draw Flattened Pixmap.vi"("image data"=w1589) -> ("new picture"=→"DragIcon":picture)  [unwired: 8 in]
        n729 = Bundle By Name(cluster=w1597, "BgIcon"=w1591, "BgIconMask"=w1592) -> (w1596:T6)
      }
      frame "ShowDragIcon", "ShowDragIcon:UpdateIcon" {
        w1637 = 2.0 ("Waveform Chart")
        w1626 = 4 ("x")
        n730 = Unbundle By Name(w1617) -> ("IconNames"=w1609:string[], "Icons"=w1649:T4[], "IconSelected"=w1608:i32, "IconPos"=w1645:T26)
        n731 = Index Array(array=w1609, index=w1608) -> (element=→"_IconName":string)
        n732 = Index Array(array=w1649, index=w1608) -> (element=w1606:T4)
        n733 = Index Array(array=w1645, index=w1608) -> (element=w1644:T29)
        n734 = property on="Icons" class="Pict"() -> ("Origin"=w1612:T17)  [unwired: 2 in, 2 out]
        n735 = Unbundle By Name(w1644) -> ("left"=w1643:i16, "top"=w1639:i16, "right"=w1642:i16, "bottom"=w1640:i16)
        n736 = call <resource>:"GDSIconEditor_ShrinkImage.vi"("image data"=w1606) -> ("image subset"=w1605:T4)  [unwired: 9 in]
        n737 = Unbundle By Name(w1605) -> ("Rectangle.right"=w1618:i16, "Rectangle.bottom"=w1619:i16)
        n738 = call <vilib>:"Draw Flattened Pixmap.vi"("image data"=w1605) -> ("new picture"=w1628:picture)  [unwired: 8 in]
        n739 = property on="Icons" class="Pict"() -> ("Position"=w1611:T15)  [unwired: 2 in, 2 out]
        n740 = Add(x=w1639, y=w1640) -> (x+y=w1638:i16)
        n741 = Add(x=w1643, y=w1642) -> (x+y=w1641:i16)
        n742 = Divide(x=w1638, y=w1637) -> (x/y=w1635:dbl)
        n743 = Divide(x=w1641, y=w1637) -> (x/y=w1636:dbl)
        n744 = Subtract(x=w1611, y=w1612) -> (x-y=w1610:T15)
        n745 = Bundle("right"=w1618, "bottom"=w1619) -> (w1627:cluster{"right":i16, "bottom":i16})  [unwired: 1 in]
        n746 = Bundle(w1636, w1635) -> (w1634:cluster{dbl, dbl})  [unwired: 1 in]
        n747 = Increment(x=w1627) -> (x+1=w1646:cluster{"right":i16, "bottom":i16})
        n748 = Add(x=w1634, y=w1610) -> (x+y=w1633:cluster{dbl, dbl})
        n749 = Divide(x=w1646, y=2.0 ("Waveform Chart")) -> (x/y=w1625:cluster{"right":dbl, "bottom":dbl})
        n750 = Multiply(x=w1626, y=w1625) -> (x*y=w1624:cluster{"right":dbl, "bottom":dbl})
        n751 = Subtract(x=w1633, y=w1624) -> (x-y=w1615:cluster{dbl, dbl})
        n752 = Multiply(x=w1626, y=w1618) -> (x*y=w1630:i32)
        n753 = Multiply(x=w1626, y=w1619) -> (x*y=w1629:i32)
        n754 = Equal?(x=w1613, y="ShowDragIcon:UpdateIcon") -> (x = y?=w1614:bool)
        n755 = Bundle(w1630, w1629) -> (w1631:cluster{i32, i32})  [unwired: 1 in]
        n756 = Select(t="UpdateIcon", s=w1614, f="Idle" ("y")) -> (s? t:f=w1620:string)
        n757 = property on="DragIcon" class="Pict"("Draw Area Size"=w1631, "Value"=w1628, "Visible"=TRUE) -> (error out=w1616:errorcluster)  [unwired: 2 in, 1 out]
        n758 = case shown="False" w1614 {
          tunnel: w1616 -> [w1651 _]
          tunnel: w1615 -> [w1650 _]
          frame False {
            n759 = property on="DragIcon" class="Pict"(error in=w1651, "Position"=w1650) -> ()  [unwired: 1 in, 2 out]
          }
          frame True {
          }
        }
      }
      frame "UpdateIconFolderList" {
        # "C:\\Users\\Mikael\\Documents\\LabVIEW Data\\Glyphs"
        n760 = VI Library() -> (path=w1666:path)
        n761 = call <resource>:"GOOP_GetGDSConfigFolder.vi"() -> ("GDSFolderPath"=w1698:path)
        n762 = call <vilib>:"Set Busy.vi"("error in (no error)"=w1680) -> ("error out"=w1679:errorcluster)  [unwired: 9 in, 1 out]
        n763 = Strip Path(path=w1666) -> (stripped path=w1678:path)  [unwired: 1 out]
        n764 = call <resource>:"GOOP_GetProviderIniFilePath.vi"() -> ("ProviderMainFolder"=w1655:path)  [unwired: 10 in, 1 out]
        n765 = Build Path(base path=w1698, name or relative path="IconFolder.txt") -> (appended path=w1687:path)
        n766 = Read from Text File(file (use dialog)=w1687) -> (text=w1696:string)  [unwired: 3 in, 3 out]
        n767 = Build Path(base path=w1678, name or relative path="resource") -> (appended path=w1667:path)
        n768 = call <vilib>:"Dflt Data Dir.vi"() -> ("App:Default Data Directory"=w1674:path)
        n769 = call <vilib>:"Trim Whitespace.vi"("string"=w1696) -> ("trimmed string"=w1683:string)  [unwired: 1 in]
        n770 = Build Path(base path=w1667, name or relative path="Framework") -> (appended path=w1668:path)
        n771 = Spreadsheet String To Array(delimiter (Tab)="\n", format string="%s", spreadsheet string=w1683, array type (2D Dbl)=string[] []) -> (array=w1661:string[])
        n772 = Build Path(base path=w1674, name or relative path="Glyphs") -> (appended path=w1675:path)
        n773 = Build Path(base path=w1668, name or relative path="Providers") -> (appended path=w1677:path)
        n774 = Build Path(base path=w1677, name or relative path="Icons") -> (appended path=w1663:path)
        n775 = Build Path(base path=w1655, name or relative path="Glyphs") -> (appended path=w1657:path)
        n776 = Build Path(base path=w1655, name or relative path="Icons") -> (appended path=w1654:path)
        n777 = Path To String(path=w1675) -> (string=w1652:string)
        n778 = Path To String(path=w1663) -> (string=w1665:string)
        n779 = Path To String(path=w1657) -> (string=w1664:string)
        n780 = Path To String(path=w1654) -> (string=w1653:string)
        n781 = Build Array(w1665, w1664, w1653, w1652) -> (w1662:string[])
        n782 = Build Array (concatenate)(w1662, w1661) -> (w1660:string[])
        n783 = for {
          tunnel: w1660 -> [w1700] mode=indexing
          tunnel: [w1703] -> w1658 mode=indexing
          tunnel: [w1699] -> w1659 mode=indexing
          n784 = String To Path(string=w1700) -> (path=w1703:path)
          n785 = String Length(string=w1700) -> (length=w1701:i32)
          n786 = Subtract(x=w1701, y=45) -> (x-y=w1702:i32)
          n787 = case shown="1.." w1702 {
            selector: w1702 -> [_ w1712]
            tunnel: w1701 -> [_ _]
            tunnel: w1700 -> [w1705 w1710]
            tunnel: [w1705 w1707] -> w1699
            frame 0, Default {
            }
            frame 1.. {
              n788 = Add(x=w1712, y=3) -> (x+y=w1709:i32)
              n789 = String Subset(string=w1710, offset (0)=w1709) -> (substring=w1708:string)  [unwired: 1 in]
              n790 = Concatenate Strings("..." ("string"), w1708) -> (w1707:string)
            }
          }
        }
        n791 = for {
          tunnel: w1658 -> [w1717] mode=indexing
          shift-right: [w1722] -> w1684
          shift-left: path[] [] -> [w1718]
          shift-right: [w1721] -> w1681
          shift-left: string[] [] -> [w1720]
          tunnel: w1659 -> [w1719] mode=indexing
          n792 = Empty String/Path?(string/path=w1717) -> (empty?=w1715:bool)
          n793 = Search 1D Array(1D array=w1718, element=w1717) -> (index of element=w1716:i32)  [unwired: 1 in]
          n794 = Greater Or Equal To 0?(x=w1716) -> (x >= 0?=w1714:bool)
          n795 = Or(x=w1715, y=w1714) -> (x .or. y?=w1713:bool)
          n796 = case shown="False" w1713 {
            tunnel: w1717 -> [w1726 _]
            tunnel: w1718 -> [w1729 w1739]
            tunnel: [w1728 w1739] -> w1722
            tunnel: w1720 -> [w1724 w1738]
            tunnel: [w1725 w1738] -> w1721
            tunnel: w1719 -> [w1723 _]
            frame False {
              n797 = call <vilib>:"Check if File or Folder Exists.vi"("path"=w1726) -> ("file or folder exists?"=w1727:bool)  [unwired: 8 in, 2 out]
              n798 = case shown="True" w1727 {
                tunnel: w1729 -> [w1731 w1737]
                tunnel: [w1731 w1736] -> w1728
                tunnel: w1726 -> [_ w1735]
                tunnel: w1724 -> [w1730 w1733]
                tunnel: [w1730 w1734] -> w1725
                tunnel: w1723 -> [_ w1732]
                frame False {
                }
                frame True {
                  n799 = Build Array (concatenate)(w1737, w1735) -> (w1736:path[])
                  n800 = Build Array (concatenate)(w1733, w1732) -> (w1734:string[])
                }
              }
            }
            frame True {
            }
          }
        }
        n801 = Build Array (concatenate)("<All icons>" ("y"), w1681) -> (w1691:string[])
        n802 = property on="_Folders" class="Ring (strict)"("Strings []"=w1691, "Value"=1) -> ()  [unwired: 2 in, 2 out]
        n803 = Bundle By Name(cluster=w1690, "Folders"=w1684) -> (w1689:T6)
      }
      frame "PlaceIcon" {
        n804 = Unbundle By Name(w1747) -> ("Icons"=w1749:T4[], "IconSelected"=w1748:i32)
        n805 = Index Array(array=w1749, index=w1748) -> (element=w1741:T4)
        n806 = call <resource>:"GDSIconEditor_ShrinkImage.vi"("image data"=w1741) -> ("image subset"=w1740:T4)  [unwired: 9 in]
        n807 = call <resource>:"GDSIconEditor_ImageDataTo8Bit.vi"("image data"=w1740) -> ("8-bit pixmap"=w1742:u8[][])  [unwired: 7 in, 3 out]
        n808 = Bundle By Name(cluster=w1747, "BgIcon"=w1742, "BgIconOffset"=cluster{"X":i32, "Y":i32} {"X"=0, "Y"=0}) -> (w1746:T6)
      }
      frame "ReadIcons" {
        (unwired) "" ("Name")
        n809 = local read "_Folders"() -> (w1752:u16)
        n810 = Unbundle By Name(w1759) -> ("Folders"=w1758:path[])
        n811 = case shown="0" w1752 {
          tunnel: w1758 -> [w1762 w1767]
          tunnel: w1752 -> [_ w1766]
          tunnel: [w1762 w1763] -> w1757
          frame 0 {
            (unwired) 0 ("index")
          }
          frame Default {
            n812 = Decrement(x=w1766) -> (x-1=w1765:u16)
            n813 = Index Array(array=w1767, index=w1765) -> (element=w1764:path)
            n814 = Build Array(w1764) -> (w1763:path[])
          }
        }
        n815 = call <vilib>:"Set Busy.vi"("error in (no error)"=w1756) -> ("error out"=w1755:errorcluster)  [unwired: 9 in, 1 out]
        n816 = for {
          tunnel: w1757 -> [w1772] mode=indexing
          shift-right: [w1768] -> w1753
          shift-left: cluster{i32, "path out":path}[] [] -> [w1769]
          shift-right: [w1773] -> w1751
          shift-left: w1755 -> [w1770]
          n817 = call <vilib>:"Check if File or Folder Exists.vi"("path"=w1772) -> ("file or folder exists?"=w1771:bool)  [unwired: 8 in, 2 out]
          n818 = case shown="True" w1771 {
            tunnel: [w1775 w1781] -> w1773
            tunnel: w1770 -> [w1775 w1780]
            tunnel: w1772 -> [_ w1779]
            tunnel: w1769 -> [w1774 w1776]
            tunnel: [w1774 w1778] -> w1768
            frame False {
            }
            frame True {
              n819 = call <vilib>:"Recursive File List.vi"("pattern"="*.png", "error in (no error)"=w1780, "Folder Path"=w1779) -> ("error out"=w1783:errorcluster, "All Files in Dir"=w1784:path[])  [unwired: 4 in, 3 out]
              n820 = for {
                tunnel: w1784 -> [w1792] mode=indexing
                tunnel: [w1790] -> w1777 mode=indexing
                shift-right: [w1789] -> w1781
                shift-left: w1783 -> [w1793]
                n821 = File/Directory Info(path=w1792, error in=w1793) -> (path out=w1791:path, size=w1788:i64, error out=w1789:errorcluster)  [unwired: 4 out]
                n822 = Divide(x=w1788, y=i64 100) -> (x/y=w1786:dbl)
                n823 = To Long Integer(number=w1786) -> (32bit integer=w1785:i32)
                n824 = Bundle(w1785, "path out"=w1791) -> (w1790:cluster{i32, "path out":path})  [unwired: 1 in]
              }
              n825 = Build Array (concatenate)(w1776, w1777) -> (w1778:cluster{i32, "path out":path}[])
            }
          }
        }
        n826 = Sort 1D Array(array=w1753) -> (sorted array=w1750:cluster{i32, "path out":path}[])
        n827 = Bundle By Name(cluster=w1759, "IconPaths"=w1750) -> (w1761:T6)
      }
      frame "DrawIcons", "DrawIcons:NoBusy" {
        w1814 = 0  # IconsPerRow
        w1818 = 10  # Border
        w1816 = 15  # Gap
        # "Y"
        # "X"
        n828 = Unbundle By Name(w1807) -> ("IconPaths"=w1799:cluster{i32, "path out":path}[])
        n829 = case shown="\"DrawIcons:NoBusy\"" w1794 {
          tunnel: w1804 -> [w1820 w1822]
          tunnel: [w1820 w1821] -> w1798
          frame "DrawIcons:NoBusy" {
          }
          frame Default {
            n830 = call <vilib>:"Set Busy.vi"("error in (no error)"=w1822) -> ("error out"=w1821:errorcluster)  [unwired: 9 in, 1 out]
          }
        }
        n831 = local read "_IconSearchText"() -> (w1797:string)
        n832 = property on="Icons" class="Pict"() -> ("Draw Area Size"=w1811:T7)  [unwired: 2 in, 2 out]
        n833 = Unbundle By Name(w1811) -> ("Width"=w1817:u32)
        n834 = property on="Icons" class="Pict"("Origin"=T17 {"Horizontal"=0, "Vertical"=0}) -> ()  [unwired: 2 in, 2 out]
        n835 = call <vilib>:"Trim Whitespace.vi"("string"=w1797) -> ("trimmed string"=w1796:string)  [unwired: 1 in]
        n836 = for {
          shift-right: [w1851] -> w1806
          shift-left: w1798 -> [w1834]
          shift-right: [w1838] -> _
          shift-left: w1818 -> [w1846]
          shift-right: [w1849] -> w1801
          shift-left: picture data[5B] ("new picture") -> [w1850]
          shift-right: [w1847] -> w1810
          shift-left: T4[] [] -> [w1848]
          shift-right: [w1839] -> _
          shift-left: w1814 -> [w1840]
          shift-right: [w1837] -> _
          shift-left: w1818 -> [w1841]
          shift-right: [w1842] -> _
          shift-left: TRUE -> [w1845]
          tunnel: w1816 -> [w1844]
          tunnel: w1817 -> [w1843]
          tunnel: w1818 -> [w1836]
          tunnel: w1799 -> [w1835] mode=indexing
          shift-right: [w1833] -> w1808
          shift-left: cluster{i32, i32, i32, i32}[] [] -> [w1832]
          shift-right: [w1830] -> w1802
          shift-left: string[] [] -> [w1831]
          tunnel: w1796 -> [w1829]
          n837 = Unbundle(w1835) -> (w1827:i32, "path out"=w1828:path)
          n838 = case shown="\"\"" w1829 {
            selector: w1829 -> [w1857 _]
            tunnel: w1828 -> [w1858 _]
            tunnel: [w1852 TRUE] -> w1824
            frame Default {
              n839 = To Lower Case(string=w1857) -> (all lower case string=w1854:string)
              n840 = call <vilib>:"Get File Extension.vi"("file"=w1858) -> ("filename without extension"=w1856:string)  [unwired: 6 in, 4 out]
              n841 = To Lower Case(string=w1856) -> (all lower case string=w1855:string)
              n842 = Match Pattern(string=w1855, regular expression=w1854) -> (offset past match=w1853:i32)  [unwired: 1 in, 3 out]
              n843 = Greater Or Equal To 0?(x=w1853) -> (x >= 0?=w1852:bool)
            }
            frame "" {
            }
          }
          n844 = Less Or Equal?(x=w1827, y=50) -> (x <= y?=w1825:bool)
          n845 = And(x=w1824, y=w1825) -> (x .and. y?=w1823:bool)
          n846 = case shown="True" w1823 {
            tunnel: w1828 -> [_ w1872]
            tunnel: w1834 -> [w1868 w1901]
            tunnel: [w1868 w1900] -> w1851
            tunnel: w1850 -> [w1867 w1899]
            tunnel: [w1867 w1878] -> w1849
            tunnel: w1848 -> [w1866 w1884]
            tunnel: [w1866 w1898] -> w1847
            tunnel: w1846 -> [w1864 w1881]
            tunnel: w1845 -> [w1862 w1897]
            tunnel: w1844 -> [_ w1883]
            tunnel: w1843 -> [_ w1894]
            tunnel: [w1862 w1893] -> w1842
            tunnel: w1841 -> [w1863 w1888]
            tunnel: w1840 -> [w1865 w1887]
            tunnel: [w1865 w1886] -> w1839
            tunnel: [w1864 w1876] -> w1838
            tunnel: [w1863 w1880] -> w1837
            tunnel: w1836 -> [_ w1882]
            tunnel: w1832 -> [w1861 w1875]
            tunnel: [w1861 w1874] -> w1833
            tunnel: w1831 -> [w1860 w1870]
            tunnel: [w1860 w1871] -> w1830
            frame False {
            }
            frame True {
              # "Place This Icon on a new row"
              n847 = call <vilib>:"Read PNG File.vi"("error in (no error)"=w1901, "path to PNG file"=w1872) -> ("error out"=w1900:errorcluster, "image data"=w1892:T4)  [unwired: 7 in, 1 out]
              n848 = Unbundle By Name(w1892) -> ("Rectangle"=w1891:T29)
              n849 = Unbundle By Name(w1892) -> ("Rectangle.right"=w1879:i16)
              n850 = Select(t=0, s=w1897, f=w1883) -> (s? t:f=w1896:i32)
              n851 = Add(x=w1896, y=w1881) -> (x+y=w1889:i32)
              n852 = Strip Path(path=w1872) -> (name=w1869:string)  [unwired: 1 out]
              n853 = Add(x=w1889, y=w1879) -> (x+y=w1885:i32)
              n854 = Greater?(x=w1885, y=w1894) -> (0:w1893:bool)
              n855 = Build Array (concatenate)(w1884, w1892) -> (w1898:T4[])
              n856 = case shown="True" w1893 {
                tunnel: [w1906 w1912] -> w1890
                tunnel: w1889 -> [w1903 _]
                tunnel: w1888 -> [w1902 w1907]
                tunnel: w1887 -> [w1905 w1915]
                tunnel: [w1904 1] -> w1886
                tunnel: w1884 -> [_ w1916]
                tunnel: w1883 -> [_ w1910]
                tunnel: w1882 -> [_ w1909]
                tunnel: w1881 -> [_ _]
                tunnel: [w1902 w1908] -> w1880
                tunnel: w1879 -> [_ _]
                frame False {
                  n857 = Bundle(w1903, "Border"=w1902, w1903, "Border"=w1902) -> (w1906:cluster{i32, "Border":i32, i32, "Border":i32})  [unwired: 1 in]
                  n858 = Increment(x=w1905) -> (x+1=w1904:i32)
                }
                frame True {
                  n859 = Delete From Array(array=w1916, length=w1915) -> (deleted portion=w1914:T4[])  [unwired: 1 in, 1 out]
                  n860 = for {
                    tunnel: w1914 -> [w1919] mode=indexing
                    tunnel: [w1918] -> w1913 mode=indexing
                    n861 = Unbundle By Name(w1919) -> ("Rectangle.bottom"=w1918:i16)
                  }
                  n862 = Array Max & Min(array=w1913) -> (max value=w1911:i16)  [unwired: 3 out]
                  n863 = Compound Arithmetic op=ADD(w1907, w1910, w1911) -> (w1908:i32)
                  n864 = Bundle("Border"=w1909, w1908, "Border"=w1909, w1908) -> (w1912:cluster{"Border":i32, i32, "Border":i32, i32})  [unwired: 1 in]
                }
              }
              n865 = Add(x=w1890, y=w1891) -> (x+y=w1873:cluster{i32, i32, i32, i32})
              n866 = Bundle By Name(cluster=w1892, "Rectangle"=w1873) -> (w1877:T4)
              n867 = Build Array (concatenate)(w1875, w1873) -> (w1874:cluster{i32, i32, i32, i32}[])
              n868 = Build Array (concatenate)(w1870, w1869) -> (w1871:string[])
              n869 = Unbundle By Name(w1877) -> ("Rectangle.right"=w1876:i16)
              n870 = call <vilib>:"Draw Flattened Pixmap.vi"("image data"=w1877, "picture"=w1899) -> ("new picture"=w1878:picture)  [unwired: 7 in]
            }
          }
        }
        "Icons" <- w1801
        n871 = property on="DragIcon" class="Pict"("Visible"=FALSE) -> ()  [unwired: 2 in, 2 out]
        n872 = Bundle By Name(cluster=w1807, "Icons"=w1810, "IconPos"=w1808, "IconNames"=w1802) -> (w1819:T6)
        n873 = call <vilib>:"Unset Busy.vi"("error in (no error)"=w1806) -> ()  [unwired: 10 in, 1 out]
      }
      frame "UpdateApplyToAllText" {
        n874 = Unbundle By Name(w1932) -> ("Counter"=w1927:i32, "VIs"=w1924:path[], "Text1"=w1921:string, "Text2"=w1920:string)
        n875 = Increment(x=w1927) -> (x+1=w1931:i32)
        n876 = Bundle By Name(cluster=w1932, "Counter"=w1931) -> (w1925:T6)
        n877 = Array Size(array=w1924) -> (size(s)=w1922:i32)
        n878 = Quotient & Remainder(x=w1927, y=2) -> (x-y*floor(x/y)=w1923:i32)  [unwired: 1 out]
        n879 = case shown="1" w1923 {
          tunnel: [w1934 w1936] -> w1928
          tunnel: w1922 -> [w1935 _]
          tunnel: w1921 -> [_ w1936]
          tunnel: w1920 -> [w1933 _]
          frame 1 {
            n880 = Format Into String(format string=w1933, w1935) -> (resulting string=w1934:string)  [unwired: 2 in, 1 out]
          }
          frame 0, Default {
          }
        }
        n881 = property on="_ApplyHeaderToAll" class="Bool (strict)"("BoolText.Text"=w1928) -> ()  [unwired: 2 in, 2 out]
      }
      frame "Exit" {
        n882 = call <resource>:"GDSError_ClearError.vi"("codes"=i32[] [1052, 8], "error in (no error)"=w1940, "Message popups"=string[] ["Invalid or too long file names!", "File permission error!"]) -> ("error out"=w1937:errorcluster)  [unwired: 15 in, 1 out]
      }
      frame "Edit header" {
        n883 = Unbundle By Name(w1963) -> ("FrameColor"=w1957:u32, "Frame thickness"=w1956:i32, "HeaderIcon"=w1955:u8[][], "Splitter0px"=w1944:bool, "Prefix"=w1945:string, "ClassBodyIcon"=w1946:string, "LibraryRef"=w1948:refnum<vi>)
        n884 = Not A Number/Path/Refnum?(number/path/refnum=w1948) -> (NaN/Path/Refnum?=w1949:bool)
        n885 = case shown="False" w1949 {
          tunnel: w1948 -> [w1966 _]
          tunnel: [w1965 enum16{"LvClass", "Library", "X-Control"}."LvClass" ("Type")] -> w1947
          frame False {
            n886 = property class="Library"(reference=w1966) -> ("Path"=w1968:path)  [unwired: 1 in, 2 out]
            n887 = call <vilib>:"Get File Extension.vi"("file"=w1968) -> ("lowercase file extension"=w1967:string)  [unwired: 6 in, 4 out]
            n888 = case shown="\"xctl\"" w1967 {
              tunnel: [enum16{"LvClass", "Library", "X-Control"}."LvClass" ("Type") enum16{"LvClass", "Library", "X-Control"}."Library" ("Type") enum16{"LvClass", "Library", "X-Control"}."X-Control" ("Type")] -> w1965
              frame "lvclass", Default {
              }
              frame "lvlib" {
              }
              frame "xctl" {
              }
            }
          }
          frame True {
          }
        }
        n889 = local read "_BackgroundColor"() -> (w1959:T2)
        n890 = Unbundle By Name(w1959) -> ("Color"=w1958:u32)
        n891 = call <resource>:"GDSIconEditor_HeaderEditorDialog.vi"("NoSplitter"=w1944, "BodyBackGround"=w1958, "HeaderText"=w1945, "error in (no error)"=w1961, "HeaderIconIn"=w1955, "Type"=w1947, "FrameThickness(1)"=w1956, "ClassBodyIcon"=w1946, "FrameColor"=w1957) -> ("NoSplitterOut"=w1943:bool, "Cancelled"=w1954:bool, "FrameColorOut"=w1953:u32, "FrameThicknessOut"=w1952:u32, "HeaderIconOut"=w1951:u8[][], "error out"=w1960:errorcluster)  [unwired: 5 in]
        n892 = case shown="False" w1954 {
          tunnel: w1960 -> [w1989 w1995]
          tunnel: [w1989 w1995] -> w1962
          tunnel: ["Generate icon" "Idle"] -> w1950
          tunnel: w1963 -> [w1992 w1993]
          tunnel: [w1991 w1993] -> w1964
          tunnel: w1953 -> [w1987 _]
          tunnel: w1952 -> [w1974 _]
          tunnel: w1951 -> [w1977 _]
          tunnel: w1943 -> [w1973 _]
          frame False {
            w1986 = u8 32 ("x")
            w1988 = TRUE
            n893 = Array Size(array=w1977) -> (size(s)=w1985:i32[])
            n894 = Index Array(array=w1985) -> (element #1=w1982:i32)  [unwired: 2 in, 1 out]
            n895 = Multiply(x=w1974, y=u8 2) -> (x*y=w1983:u32)
            n896 = Equal To 0?(x=w1982) -> (x = 0?=w1981:bool)
            n897 = Add(x=w1982, y=w1983) -> (x+y=w1979:u32)
            n898 = Increment(x=w1979) -> (x+1=w1980:u32)
            n899 = Select(t=w1979, s=w1981, f=w1980) -> (s? t:f=w1978:u32)
            n900 = Subtract(x=w1986, y=w1978) -> (x-y=w1976:u32)
            n901 = Subtract(x=w1986, y=w1983) -> (x-y=w1975:u32)
            n902 = Bundle By Name(cluster=w1992, "Splitter0px"=w1973, "Header exists"=w1988, "Icon exist"=w1988, "FrameColor"=w1987, "Frame thickness"=w1974, "HeaderIcon"=w1977, "BodyIconHeight"=w1976, "BodyIconWidth"=w1975) -> (w1991:T6)
          }
          frame True {
            # "Cancel"
          }
        }
      }
      frame "Edit Library Header" {
        # "Cancel"
        n903 = Unbundle By Name(w2002) -> ("LibraryRef"=w1998:refnum<vi>)
        n904 = call <resource>:"GDSLvIcon_DialogUpdateClass.vi"("ClassPath(FilePath/ProjectTreePath/LvCLassRef)"=w1998, "error in (no error)"=w2000) -> ("Splitter0px"=w1996:bool, "error out"=w2001:errorcluster)  [unwired: 13 in, 3 out]
        n905 = Bundle By Name(cluster=w2002, "Splitter0px"=w1996) -> (w1997:T6)
      }
      frame "Apply icon" {
        n906 = Unbundle By Name(w2011) -> ("IconOut"=w2022:u8[][], "ViRef"=w2021:refnum<vi>)  [unwired: 2 out]
        n907 = Unbundle By Name(w2011) -> ("StartIconSize"=w2012:u16)
        n908 = local read "_IconSize"() -> (w2004:u16)
        n909 = Reshape Array(w2022, 1024 ("dimension size")) -> (w2017:u8[])
        n910 = Bundle By Name(cluster=T4 {"image type"=0, "image depth"=8, "image"=[], "mask"=[], "colors"=[], "Rectangle"={"left"=0, "top"=0, "right"=32, "bottom"=32}} ("image data"), "image"=w2017) -> (w2018:T4)
        n911 = Not Equal?(x=w2012, y=w2004) -> (x != y?=w2010:bool)
        n912 = invoke class="VI" method="VI Icon.Set from Image Data"(reference=w2021, error in=w2023, "ImageData"=w2018) -> (reference out=w2005:refnum<vi>, error out=w2007:errorcluster)  [unwired: 3 in, 4 out]
        n913 = case shown="True" w2010 {
          tunnel: w2007 -> [w2025 w2030]
          tunnel: [w2025 w2029] -> w2009
          tunnel: w2005 -> [w2024 w2028]
          tunnel: w2004 -> [_ w2027]
          tunnel: [w2024 w2026] -> w2003
          frame False {
          }
          frame True {
            # "We also need to rewire the connector Pane Controls"
            n914 = call <resource>:"GOOP_GetControlRearrangement.vi"("VI Refnum"=w2028, "_IconSize"=w2027, "error in (no error)"=w2030) -> ("ControlsToMove"=w2031:T22, "error out"=w2032:errorcluster)  [unwired: 10 in, 5 out]
            n915 = property class="VI"(reference=w2028, error in=w2032) -> (reference out=w2026:refnum<vi>, error out=w2033:errorcluster, "ConPane"=w2037:refnum<vi>)
            n916 = for {
              tunnel: w2031 -> [w2041] mode=indexing
              tunnel: w2037 -> [w2043]
              shift-right: [w2039] -> w2035
              shift-left: w2033 -> [w2042]
              tunnel: [w2038] -> w2034 mode=indexing
              n917 = Unbundle By Name(w2041) -> ("CtrlRef"=w2038:refnum<vi>, "AfterTerminalIndex"=w2040:i32)
              n918 = invoke class="ConPane" method="AssignCtrlToTerm"(reference=w2043, error in=w2042, "Control"=w2038, "TermIdx"=w2040) -> (error out=w2039:errorcluster)  [unwired: 1 in, 4 out]
            }
            n919 = Close Reference(reference=w2034, error in (no error)=w2035) -> (error out=w2036:errorcluster)
            n920 = Close Reference(reference=w2037, error in (no error)=w2036) -> (error out=w2029:errorcluster)
          }
        }
        n921 = local read "_ApplyHeaderToAll"() -> (w2016:bool)
        n922 = Select(t="ApplyToAll", s=w2016, f="Exit" ("item tag")) -> (s? t:f=w2015:string)
        n923 = call <resource>:"Scripting_SaveVi.vi"("ForceResaving(False)"=TRUE, "error in (no error)"=w2009, "VIRefToSaveIn"=w2003) -> ("error out"=w2008:errorcluster)  [unwired: 7 in, 1 out]
      }
      frame "ApplyToAll" {
        n924 = Unbundle By Name(w2052) -> ("AppRef"=w2045:refnum<vi>, "VIs"=w2053:path[])
        n925 = Unbundle By Name(w2052) -> ("FrameColor"=w2051:u32, "Frame thickness"=w2050:i32, "HeaderIcon"=w2049:u8[][], "Splitter0px"=w2044:bool)
        n926 = for {
          tunnel: w2053 -> [w2075] mode=indexing
          tunnel: w2051 -> [w2072]
          tunnel: w2050 -> [w2071]
          tunnel: w2049 -> [w2070]
          shift-right: [w2058] -> w2047
          shift-left: w2048 -> [w2058]
          tunnel: w2045 -> [w2055]
          tunnel: w2044 -> [w2054]
          # "Ignore error since file coudl be read only"
          n927 = call <resource>:"Scripting_OpenViRef.vi"("error in"=w2058, "ViPath/ViName/Viref"=w2075, "AppRef"=w2055) -> ("error out"=w2074:errorcluster, "vi reference"=w2057:refnum<vi>)  [unwired: 6 in, 1 out]
          n928 = call <resource>:"GDSLvIcon_AnalyseViIcon.vi"("ViRef/LvCLassRef/LvLibRef/ViPath/2D_Image"=w2057, "error in (no error)"=w2074) -> ("BodyIcon"=w2069:u8[][], "error out"=w2073:errorcluster)  [unwired: 4 in, 12 out]
          n929 = call <resource>:"GDSLvIcon_CreateIconPicture.vi"("FrameColor"=w2072, "FrameThickness(1)"=w2071, "HeaderIconIn"=w2070, "BodyIconIn"=w2069, "error in (no error)"=w2073, "0px Splitter(False)"=w2054) -> ("WholeIconOut"=w2060:u8[][], "error out"=w2059:errorcluster)  [unwired: 8 in, 4 out]
          n930 = Reshape Array(w2060, 1024 ("dimension size")) -> (w2065:u8[])
          n931 = Bundle By Name(cluster=T4 {"image type"=0, "image depth"=8, "image"=[], "mask"=[], "colors"=[], "Rectangle"={"left"=0, "top"=0, "right"=32, "bottom"=32}} ("image data"), "image"=w2065) -> (w2067:T4)
          n932 = invoke class="VI" method="VI Icon.Set from Image Data"(reference=w2057, error in=w2059, "ImageData"=w2067) -> (reference out=w2063:refnum<vi>, error out=w2064:errorcluster)  [unwired: 3 in, 4 out]
          n933 = call <resource>:"Scripting_SaveVi.vi"("ForceResaving(False)"=TRUE, "error in (no error)"=w2064, "VIRefToSaveIn"=w2063) -> ("error out"=w2061:errorcluster, "VIRefToSaveOut"=w2062:refnum<vi>)  [unwired: 7 in]
          n934 = Close Reference(reference=w2062, error in (no error)=w2061) -> ()  [unwired: 1 out]
        }
      }
      frame "Template VI" {
        (unwired) T30."existing file (use LLBs)" ("select mode (2)")
        n935 = File Dialog(6:"*.vi;*.ctl;*.vit;*.ctt;*.llb", 7:"Select template VI" ("prompt")) -> (1:w2084:bool, 2:w2083:bool, 3:w2078:path)  [unwired: 5 in, 1 out]
        n936 = Compound Arithmetic op=AND(w2083, invert w2084) -> (w2082:bool)
        n937 = case shown="True" w2082 {
          tunnel: w2081 -> [w2089 w2094]
          tunnel: [w2089 w2093] -> w2080
          tunnel: ["Idle" w2099] -> w2079
          tunnel: w2078 -> [_ w2095]
          tunnel: w2077 -> [w2087 w2097]
          tunnel: [w2087 w2104] -> w2076
          frame False {
            # "Cancel"
          }
          frame True {
            n938 = Unbundle By Name(w2097) -> ("AppRef"=w2096:refnum<vi>)
            n939 = Open VI Reference(application reference (local)=w2096, vi path=w2095, options=2, error in (no error)=w2094) -> (vi reference=w2091:refnum<vi>, error out=w2093:errorcluster)  [unwired: 2 in]
            n940 = call <resource>:"GDSLvIcon_AnalyseViIcon.vi"("ViRef/LvCLassRef/LvLibRef/ViPath/2D_Image"=w2091, "error in (no error)"=w2093) -> ("Splitter0px"=w2090:bool, "FrameColor"=w2102:u32, "FrameThickness(1)"=w2101:u32, "ValidHeaderIcon"=w2103:bool, "HeaderIcon"=w2100:u8[][], "error out"=w2092:errorcluster)  [unwired: 4 in, 8 out]
            n941 = Close Reference(reference=w2091, error in (no error)=w2092) -> ()  [unwired: 1 out]
            n942 = case shown="True" w2103 {
              tunnel: w2097 -> [w2107 w2125]
              tunnel: [w2107 w2124] -> w2104
              tunnel: w2102 -> [_ w2123]
              tunnel: w2101 -> [_ w2111]
              tunnel: w2100 -> [_ w2112]
              tunnel: ["Idle" "Generate icon"] -> w2099
              tunnel: w2090 -> [_ w2108]
              frame False {
                n943 = One Button Dialog(message="No header found in vi.") -> ()  [unwired: 1 in, 1 out]
              }
              frame True {
                w2120 = u8 32 ("x")
                w2122 = TRUE
                n944 = Array Size(array=w2112) -> (size(s)=w2119:i32[])
                n945 = case shown="True" w2108 {
                  tunnel: [w2127 w2129] -> w2118
                  tunnel: w2111 -> [w2126 w2129]
                  frame False {
                    n946 = Multiply(x=w2126, y=u8 2) -> (x*y=w2127:u32)
                  }
                  frame True {
                  }
                }
                n947 = Index Array(array=w2119) -> (element #1=w2117:i32)  [unwired: 2 in, 1 out]
                n948 = Equal To 0?(x=w2117) -> (x = 0?=w2116:bool)
                n949 = Add(x=w2117, y=w2118) -> (x+y=w2114:u32)
                n950 = Increment(x=w2114) -> (x+1=w2115:u32)
                n951 = Select(t=w2114, s=w2116, f=w2115) -> (s? t:f=w2113:u32)
                n952 = Subtract(x=w2120, y=w2113) -> (x-y=w2110:u32)
                n953 = Subtract(x=w2120, y=w2118) -> (x-y=w2109:u32)
                n954 = Bundle By Name(cluster=w2125, "Header exists"=w2122, "Icon exist"=w2122, "FrameColor"=w2123, "Frame thickness"=w2111, "HeaderIcon"=w2112, "BodyIconHeight"=w2110, "BodyIconWidth"=w2109, "Splitter0px"=w2108) -> (w2124:T6)
              }
            }
          }
        }
      }
      frame "Error" {
        n955 = call <resource>:"GDSError_LogErrorInformation.vi"("State"=w2132, "LocalVariableData"=w2130, "error in (no error)"=w2131) -> ()  [unwired: 16 in, 1 out]
      }
    }
    n956 = Equal?(x=w69, y="Exit") -> (x = y?=w73:bool)
    n957 = Select(t="Error" ("y"), s=w71, f=w69) -> (s? t:f=w70:string)
  }
  "error out" <- w23
  n958 = property class="VI"("Front Panel.WinBounds"=w32) -> ()  [unwired: 2 in, 2 out]
  n959 = Release Queue(queue=w39) -> ()  [unwired: 2 in, 3 out]
  n960 = Unbundle By Name(w49) -> ("ViRef"=w48:refnum<vi>, "LibraryRef"=w41:refnum<vi>)
  n961 = stacked-sequence {
    tunnel: w23 -> [_]
    frame #0 {
      w2135 = FALSE ("Boolean Text.Font:Bold")
      n962 = property on="_OCR" class="Bool (strict)"("BoolText.FontBold"=w2135, "BoolText.FontUnder"=w2135, "Visible"=FALSE) -> ()  [unwired: 2 in, 2 out]
    }
  }
  n963 = Close Reference(reference=w41) -> (error out=w42:errorcluster)  [unwired: 1 in]
  n964 = case shown="True" w43 {
    tunnel: w48 -> [w2136 w2138]
    tunnel: [w2136 _] -> _
    tunnel: w42 -> [_ _]
    tunnel: [_ FALSE ("Visible")] -> w29
    frame False {
    }
    frame True {
      n965 = Close Reference(reference=w2138) -> ()  [unwired: 1 in, 1 out]
    }
  }
  n966 = property on="DragIcon" class="Pict"("Visible"=w29) -> ()  [unwired: 2 in, 2 out]
